vi "MainProgram.vi"(0 "DAQmx Task":refnum<k21>, 1 "BNC Port":refnum<visa-resource-name>, 2 "SRS Port":refnum<visa-resource-name>, 3 "Energy Meter  port":refnum<visa-resource-name>, 4 "SDG II port":refnum<visa-resource-name>, 5 "Mode":T18=enum."GenericTOF", 6 "Micos Port":refnum<visa-resource-name>="COM3", 7 "CommPort (ESP300)":refnum<visa-resource-name>="COM7", 8 "Serial Config (Micos)":T15={"Baud Rate"=115200, "Parity"=0, "Data Bits"=8, "Stop Bits"=10, "Flow Control"=0} {"Flow Control" items=["None", "XON/XOFF", "RTS/CTS", "XON/XOFF & RTS/CTS", "DTR/DSR", "XON/XOFF & DTR/DSR"]; "Stop Bits" items=["1.0"=10, "1.5"=15, "2.0"=20]; "Data Bits" items=["7"=7, "8"=8]; "Parity" items=["None", "Odd", "Even", "Mark", "Space"]; "Baud Rate" items=["300"=300, "600"=600, "1200"=1200, "2400"=2400, "4800"=4800, "9600"=9600, "19200"=19200]}, 9 "Serial Config (ESP300)":T15={"Baud Rate"=19200, "Parity"=0, "Data Bits"=8, "Stop Bits"=10, "Flow Control"=2} {"Flow Control" items=["None", "XON/XOFF", "RTS/CTS", "XON/XOFF & RTS/CTS", "DTR/DSR", "XON/XOFF & DTR/DSR"]; "Stop Bits" items=["1.0"=10, "1.5"=15, "2.0"=20]; "Data Bits" items=["7"=7, "8"=8]; "Parity" items=["None", "Odd", "Even", "Mark", "Space"]; "Baud Rate" items=["300"=300, "600"=600, "1200"=1200, "2400"=2400, "4800"=4800, "9600"=9600, "19200"=19200]}, 10 "#Axis (Micos)":i32=3, 11 "#Axis (ESP300)":i32=3, 12 "Simulation (Micos)":bool=TRUE, 13 "Simulation (ESP300)":bool=TRUE, 14 "MainDAQ_Selector":T16=enum."FakeSignal(Emulator)" caption="Restart Required", 15 "Laser Control Method":T17=enum."SDG_II" caption="Restart Required") -> ()   [LabVIEW 2013]
uses:
  Files/Signal_Segment.ctl
  ControlDef/ProcessingMode.ctl
  ControlDef/Average#.ctl
  ProcessMethods/Binning/BinType.ctl
  ControlDef/MainDAQ_Selector.ctl
  ControlDef/LaserCtrl_Method.ctl
  ControlDef/SpecLengthSelector.ctl
  ControlDef/SampleRateSelector.ctl
  ControlDef/DAQRangeSelector.ctl
  <instrlib>/DG535/Command/DG535_TriggerMode.ctl
  ControlDef/StepWidthSelector.ctl
  ControlDef/Files_Format.ctl
  <instrlib>/DG535/DG535_Configs.ctl
  <instrlib>/DG535/Command/Set Trigger.ctl
  <instrlib>/DG535/Command/Set Delay.ctl
  <instrlib>/DG535/Command/DG535_Channel.ctl
  <instrlib>/DG535/Command/Set Output.ctl
  <instrlib>/DG535/Command/DG535_Output.ctl
  <instrlib>/AnalogDiscSDKLv/VIs/DWF_AnalogIn_Configurations.ctl
  <instrlib>/AnalogDiscSDKLv/VIs/DWF_AcqMode.ctl
  <instrlib>/AnalogDiscSDKLv/VIs/DWF_Filter.ctl
  <instrlib>/AnalogDiscSDKLv/VIs/DWF_TrigSrc.ctl
  <instrlib>/AnalogDiscSDKLv/VIs/DWF_TrigCond.ctl
  <instrlib>/AnalogDiscSDKLv/VIs/DWF_TrigType.ctl
  <instrlib>/GageLv_uic/VI/Gage_Configs.ctl
  ControlDef/InstruMode_Typedef.ctl
  Hardware/BNC(QuantumComposers)/BNC_Configs.ctl
  ControlDef/InstrumentSpecificControls/UIC-AToF/InitializationParams_BNC565_2Ch_AToF.ctl
  Hardware/BNC(QuantumComposers)/Command/Set C-Input.ctl
  Hardware/BNC(QuantumComposers)/Command/Set C-Mode.ctl
  Hardware/BNC(QuantumComposers)/Command/Set C-Output.ctl
  Hardware/BNC(QuantumComposers)/Command/Set C-Enable.ctl
  <instrlib>/GenericDAQ/VI/GenericDAQ_Configs.ctl
  <vilib>/Utility/error.llb/DialogType.ctl
  ControlDef/AllControlsRefs.ctl
  ControlDef/States-AToF.ctl
  Hardware/FemtoLaser(Legacy)/Laser_Status.ctl
  Files/SaveControlsRef.ctl
  Files/WriterState.ctl
  Hardware/DAQmx(Legacy)/DAQmx_Status.ctl
  Hardware/EPM2000(Legacy)/EPM2K_Status.ctl
  ProcessMethods/SignalAverager/ProcessParams.ctl
  ProcessMethods/SignalAverager/DAQParams.ctl
  ProcessMethods/SignalAverager/DisplayGraph.ctl
  <instrlib>/ESP300/Public/Data/ESP300_State.ctl
  Hardware/BNC(QuantumComposers)/BNC_States.ctl
  <instrlib>/DG535/Command/DG535_States.ctl
  <instrlib>/Micos_uic/Public/Data/Micos_Data.ctl
  ControlDef/QueueRefs.ctl
  <instrlib>/AnalogDiscSDKLv/VIs/DWF_CtrlQueue.ctl
  <instrlib>/AnalogDiscSDKLv/VIs/DWF_State.ctl
  ControlDef/Signal.ctl
  ProcessMethods/SignalAverager/ProcessStates.ctl
  <instrlib>/AnalogDiscSDKLv/VIs/DWF_Signal.ctl
  <instrlib>/AnalogDiscSDKLv/VIs/DWF_PrivateStats.ctl
  <instrlib>/AnalogDiscSDKLv/VIs/DWF_InstrumentStatus.ctl
  <instrlib>/GageLv_uic/VI/Gage_PrivateStats.ctl
  <instrlib>/GageLv_uic/VI/Gage_DAQStatus.ctl
  Apps/GenericUSBCamera/CameraEventTypedef.ctl
  Hardware/Joystick/Joystick_UserEvent.ctl
  <instrlib>/GenericDAQ/VI/GenericDAQ_PrivateStats.ctl
  <instrlib>/GenericDAQ/VI/GenericDAQ_Status.ctl
  <instrlib>/GageLv_uic/VI/SetSecondaryDataVIRef_Typedef.ctl
  Files/BinaryHeader.ctl
  Apps/BeamProfiling/BeamProfiling_Params.ctl
  Apps/ImagingMS/Imaging_Params.ctl
  <instrlib>/Micos_uic/Public/Data/Micos_State.ctl
  <vilib>/Analysis/baseanly.llb/A x Vector.vi
  ControlDef/QuitProg.vi
  <instrlib>/Micos_uic/Public/Position_Micos.vi
  <instrlib>/ESP300/Public/Position_ESP300.vi
  ControlDef/MiscParams.vi
  ControlDef/PauseMeander.vi
  <userlib>/_OpenG.lib/comparison/comparison.llb/DBL Changed__ogtk.vi
  UI/Autoscale_Y_Single.vi
  <vilib>/Analysis/Matrix/Numeric/Conversions/Array To Matrix - RA2.vi
  <instrlib>/DG535/SRS_DG535_Lib.lvlib
  <instrlib>/ESP300/ESP300.lvlib
  <instrlib>/Micos_uic/Micos_uic.lvlib
  <userlib>/Utility/ErrorLog_lib.lvlib
  Hardware/Signal_Emulator(Legacy)/Emu_CoreDAQ_Globle.vi
  <instrlib>/AnalogDiscSDKLv/AnalogDiscSDKLv.lvlib
  <instrlib>/GageLv_uic/Gage.lvlib
  <vilib>/userdefined/High Color/IMAQdx.ctl
  <vilib>/Analysis/Matrix/NI_Matrix.lvlib
  <vilib>/Analysis/NI_AALBase.lvlib
  <instrlib>/GenericDAQ/GenericDAQ.lvlib
panel:
  out "Graph (B)":cluster{dbl[], dbl[]}(graph) caption="ChiMS, (C) 2014, Laser Ablation Time-of-Flight Mass Spectrometer with Postionization, under LGPLv3 license, rev.1845"
  in  "Scale(B)Y--":bool caption="AutoScale Y"
  in  "Scale(B)Y++":bool caption="AutoScale Y"
  in  "Binning(B)":bool
  in  "IncrementUpdate(B)":bool=TRUE caption="Increment"
  in  "Scale(B)X++":bool caption="AutoScale X"
  in  "Scale(B)X--":bool caption="AutoScale X"
  in  "Scale(B)_X":bool caption="AutoScale X"
  in  "GraphEnable (B)":bool=TRUE caption="Graph (B)"
  in  "Scale(B)_Y":bool caption="AutoScale Y"
  in  "SW_Average":T1=10 caption="Average" items=["1"=1, "5"=5, "10"=10, "25"=25, "50"=50, "100"=100, "250"=250, "500"=500, "1000"=1000, "2500"=2500, "5000"=5000]
  out "Graph (A)":cluster{dbl[], dbl[]}(graph)
  in  "Scale(A)Y--":bool caption="AutoScale Y"
  in  "Scale(A)Y++":bool caption="AutoScale Y"
  in  "Binning(A)":bool
  in  "IncrementUpdate(A)":bool caption="Increment"
  in  "Scale(A)X++":bool caption="AutoScale X"
  in  "Scale(A)X--":bool caption="AutoScale X"
  in  "Scale(A)_X":bool caption="AutoScale X"
  in  "Scale(A)_Y":bool caption="AutoScale Y"
  in  "GraphEnable (A)":bool=TRUE caption="Graph (A)"
  out "Nd:YAG Energy":dbl(slide) caption="Nd:YAG Energy (J)" scale=0.0..0.03 scale format="%#_2p"
  out "LaserEnergy":dbl(slide) caption="Spitfire Energy (J)" scale=0.0..2e-06 scale format="%#_2p"
  in  "LaserON":bool caption="Spitfire"
  in  "Files Format":T2=enum."Binary Files"
  in  "Snap":bool
  in  "Record":bool
  in  "Signal Segment":T3={"SampleRate"=1000000000.0, "TrigDelay"=0.0, "SpecLength"=512.0, "DAQ_Range"=1000.0, "Average#"=0, "Position"=[], "Spectrum"=[], "Calibr."=[], "Pressure"=-1.0, "Desp_LaserEnergy"=0.0, "PI_LaserEnergy"=0.0, "Voltages Table"=[[0.0, 0.0, 0.0, 0.0]], "ProcMode"=enum."None", "Threshold"=0.005, "Comment"="", "TickCount"=0.0, "Time Stamp"=timestamp(0 s since 1904-01-01)} {"TickCount" format="%#.2f"}
  in  "Setting Panel":T5(tab)=enum."Com.Setup"
  in  "Pause":bool
  in  "StepWidth (Micos)":T6=0.2 caption="StepWidth" items=["0.2 um"=0.0002, "0.001 mm"=0.001, "0.002 mm"=0.002, "0.005 mm "=0.005, "0.01 mm"=0.01, "0.02 mm"=0.02, "0.05 mm"=0.05, "0.1 mm"=0.1, "0.2 mm"=0.2, "1 mm"=1.0]
  in  "SetFocus":bool caption="Go To"
  in  "Focus (-)":bool
  in  "Focus (+)":bool
  in  "Back(+)":bool
  in  "Front(-)":bool
  in  "Back":bool
  in  "Front":bool
  in  "Down(-)":bool
  in  "Right(-)":bool
  in  "Up(+)":bool
  in  "Left(+)":bool
  in  "Right":bool
  in  "Left":bool
  in  "StopMoving":bool
  in  "Up":bool
  in  "Down":bool
  in  "Home(Micos)":bool
  in  "MoveAbs(Micos)":bool caption="Go To"
  in  "Destination":dbl[](array[numeric])=[17.0, 17.0, 24.2] caption="Destination (mm)" min=0.0 max=34.0 format="%#.5f"
  in  "Meander":bool
  in  "Accele.(Micos)":dbl=20.0 caption="Acceleration" format="%#.3f"
  in  "Velocity(Micos)":dbl=10.0 caption="Velocity" format="%#2.3f"
  out "Velcoty_ind_micos":dbl=10.0 caption="Velocity" format="%#_5f"
  out "Accele._ind_micos":dbl=20.0 caption="Acceleration" format="%#_4f"
  out "Position(Micos)":dbl[](array[numeric]) caption="Stage Position (mm)" format="%#.5f"
  in  "DepthProfile":bool
  in  "BeamProfiling(ESP)":bool
  in  "Velocity (ESP) #3":dbl=2.0 caption="Velocity#3" format="%#.3g"
  in  "DelayScan":bool
  in  "MotorDisabled(ESP)":bool
  in  "Meander (ESP)":bool
  in  "Accele. (ESP)":dbl=0.8 caption="Acceleration" format="%#.3g"
  in  "Set dbl pulse Delay":bool
  in  "DP_Delay (ps)":dbl caption="Delay (ps)" min=-3.0 max=300.0 format="%#.3f"
  in  "Down(ESP)":bool
  in  "Up(ESP)":bool
  in  "STOP(ESP)":bool
  in  "Left(ESP)":bool
  in  "Right(ESP)":bool
  in  "Destination(ESP)":dbl[](array[numeric])=[0.0, 0.25, 32.7] caption="Destination" min=0.0 max=360.0 format="%.4f"
  in  "Go(ESP)":bool
  in  "HomeSearch(ESP)":bool
  in  "Velocity (ESP)":dbl=0.2 caption="Velocity" format="%#.3g"
  out "Position(ESP)":dbl[](array[numeric]) caption="Currrent Postion"
  in  "StepWidth (ESP)":T6=0.1 caption="StepWidth (mm)" items=["0.2 um"=0.0002, "0.001 mm"=0.001, "0.002 mm"=0.002, "0.005 mm "=0.005, "0.01 mm"=0.01, "0.02 mm"=0.02, "0.05 mm"=0.05, "0.1 mm"=0.1, "0.2 mm"=0.2, "1 mm"=1.0]
  in  "ZeroDelayPos":dbl=0.679 caption="0 Delay@(mm)" format="%#.3f"
  out "DP_Delay (ps)_indicator":dbl caption="Delay (ps)" min=-3.0 max=300.0 format="%#.3f"
  in  "Delay(PI)":dbl=3e-05 caption="VUV Delay" min=-0.001 max=0.001 step=1e-08 format="%_3ps"
  in  "Delay(LDI-Rej.)":dbl=-2e-06 caption="LDIRej_end" min=-0.001 max=0.0 step=1e-07 format="%_3ps"
  in  "SRS On/Off":bool caption="Dont Rely On\nShowing\nCheck BNC"
  in  "Internal/Burst Rate":dbl=10.0 caption="Internal/Burst Rate (Hz)" min=0.001 max=1000000.0 format="%.3f"
  in  "Trigger Mode (SRS)":T7=enum."External" caption="Trigger Mode"
  in  "Ch_D":dbl=2.8e-05 format="%_3ps"
  in  "Ch_C":dbl format="%_3ps"
  in  "Ch_B":dbl=3e-05 format="%_3ps"
  in  "Ch_A":dbl=0.099807701 format="%_7ps"
  in  "Width B":dbl=1e-06 min=0.0 max=9.9e-05 step=1e-09 format="%_3ps"
  in  "Width A":dbl=1e-06 min=0.0 max=9.9e-05 step=1e-09 format="%_3ps"
  in  "BNC On/Off":bool caption="Dont Rely On\nShowing\nCheck BNC"
  in  "Mode (BNC)":T8(ring)=enum."Single Shot" caption="Mode"
  in  "Channels Enable Status":bool[](array[boolean])=[TRUE, TRUE]
  in  "Set Mode":bool caption="Set BNC"
  in  "Trigger Mode (BNC)":T9(ring)=enum."Triggered" caption="Trigger Mode"
  in  "Rep.Rate (BNC)":dbl=10.0 caption="Repetive Rate" min=0.0 max=1000.0 format="%#_6f Hz"
  in  "Delay B":dbl min=0.0 max=9.9e-05 step=1e-09 format="%_3ps"
  in  "Delay A":dbl format="%_3ps"
  in  "Gain (Voltage Range)":T10=4294966296 items=["-100~900 mV"=4294966296, "-380~20 mV"=4294966895, "-20~380 mV"=4294966896, "+/-5 V"=10000, "+/-2 V"=4000, "+/-1 V"=2000, "+/-500 mV"=1000, "+/-200 mV"=400, "+/-100 mV"=200, "+/-50 mV"=100]
  in  "Spectrum Length":T11=32768.0 items=["256K"=262144.0, "192K"=196608.0, "128K"=131072.0, "96K"=98304.0, "64K"=65280.0, "32K"=32768.0, "24K"=24576.0, "16K"=16384.0, "8K"=8192.0, "1K"=1024.0, "512"=512.0]
  in  "SampleRate":T12=500000000.0 items=["50MS/s"=50000000.0, "100MS/s"=100000000.0, "125MS/s"=125000000.0, "200MS/s"=200000000.0, "250MS/s"=250000000.0, "500MS/s"=500000000.0, "1GS/s"=1000000000.0, "1.6GS/s"=1600000000.0]
  in  "Threshold":dbl=0.01 format="%#_3pV"
  in  "Baseline":dbl
  in  "TopLine":dbl=1.0
  in  "Processing Mode":T4
  in  "ZeroOffsetCorrection":dbl=0.0055 format="%.3p V"
  in  "Resolution(B)":bool
  in  "Resolution(A)":bool
  in  "Cali.":dbl[](array[numeric])=[0.0707, 0.16163, 0.02539] caption="Calibration Params (a, b, c)" format="%#.6f"
  in  "Switch(SDG_II)":bool caption="Status"
  in  "Mode(SDG_II)":bool caption="Mode"
  in  "ManlTrig(SDG)":bool caption="Manual Trigger"
  in  "BinWidth (A)":dbl=0.1
  in  "BinType (A)":T13=enum."ByMass"
  in  "BinWidth (B)":dbl=0.5
  in  "BinType (B)":T13=enum."ByScreen"
  in  "DisplayIncrement":u32=15
  in  "YAGEnergyCoeff.":dbl=132.6
  in  "fsEnergyCoeff.":dbl=1.29
  in  "GenericDAQ_Config":T14={"Acquisition"={"Sample Rate"=1000000000.0, "Mode"=0, "Start (0)"=0.0, "Depth"=1024.0, "Segment"=1}, "Channels"=[{"Range"=1, "DC Offset"=0}], "Mode(Gage)"=enum."Continuous"} {"Acquisition"."Depth" min=256.0 step=128.0; "Acquisition"."Mode" items=["Single", "Dual", "Quad", "Octal"]; "Acquisition"."Sample Rate" format="%.0p"}
  out "Filename Indicator":path caption="Filename"
  in  "ComSettingsTab":enum32{"Micos", "ESP300", "Misc", "Misc 2"}(tab)=enum."ESP300"
  in  "ColdStartReset":bool=TRUE caption="ResetSettings"
  in  "Gage_Config":T19={"Acquisition"={"Sample Rate"=500000000.0, "Mode"=0, "Start (0)"=0.0, "Depth"=32768.0, "Segment Size"=32768.0, "Trigger Delay"=0.0, "Trigger Timeout"=-1.0, "Trigger Holdoff"=0.0, "Clock mode"=enum."Internal", "Segment"=1}, "Channels"=[{"Coupling"=1, "Differential Input"=FALSE, "Direct-to-ADC"=FALSE, "Range"=2000, "Impedance"=50, "DC Offset"=0, "Filter"=0}], "Trigger"={"Slope"=1, "Level"=25, "Source"=0, "External Range"=10000, "External Coupling"=0, "External"=TRUE, "Disable"=FALSE, "External Impedance"=0}, "Mode(Gage)"=enum."Continuous"} {"Trigger"."External Impedance" items=["50 Ohm", "HiZ"]; "Trigger"."External Coupling" items=["DC", "AC"]; "Trigger"."External Range" min=2000 max=10000 step=8000; "Trigger"."Slope" items=["Rising", "Falling"]; "Trigger"."Level" min=-100 max=100; "Trigger"."Source" min=0 max=64 step=1; "Channels"."Impedance" min=50 max=1000000 step=999950; "Channels"."Coupling" items=["DC", "AC"]; "Acquisition"."Segment Size" min=256.0 step=128.0; "Acquisition"."Trigger Delay" min=0.0 step=128.0; "Acquisition"."Trigger Timeout" format="%.0p"; "Acquisition"."Trigger Holdoff" min=0.0 step=128.0; "Acquisition"."Depth" min=256.0 step=128.0; "Acquisition"."Mode" items=["Single", "Dual", "Quad", "Octal"]; "Acquisition"."Sample Rate" format="%.0p"}
  in  "AnalogDisc_Configs":T20={"Acqusition"={"Freq(Hz,SampleRate)"=10000000.0, "BufferSize"=8192, "Mode"=enum."Single", "RecordLength(s)"=8192.0}, "Channels"=[{"Range(V)"=5.0, "Offset(V)"=0.0, "Filter"=enum."Decimate", "Enable"=TRUE}], "Trigger"={"TriggerSource"=enum."None", "Timeout(s)"=0.0, "Holdoff(s)"=1e-06, "Position(s)"=0.0}, "AnalogTrigger"={"Channel"=0, "Polarity"=enum."Rising", "Type"=enum."Pulse", "Level(V)"=0.0, "Filter"=enum."Decimate", "Hysterisis(V)"=0.0}} {"AnalogTrigger"."Hysterisis(V)" format="%#_6p"; "Acqusition"."RecordLength(s)" format="%#_6p"; "Acqusition"."Freq(Hz,SampleRate)" format="%#_6p"; "Acqusition"."BufferSize" min=1 max=16384 step=1; "Trigger"."Position(s)" format="%#_6p"; "Trigger"."Holdoff(s)" format="%#_6p"}
  in  "Timing Tab":enum32{"DG535", "BNC"}(tab)
  in  "DG535_Configs":T26={"Trigger"={"Trigger Mode"=enum."External", "Internal/Burst Rate"=10.0, "External  Level"=1.5, "Impedance"=TRUE, "Slope"=FALSE}, "Delays"=[{"Channel"=enum."A Output", "Sync To"=enum."T0 Output", "Delay"=0.099807701}, {"Channel"=enum."B Output", "Sync To"=enum."A Output", "Delay"=1.2e-05}, {"Channel"=enum."C Output", "Sync To"=enum."T0 Output", "Delay"=0.0}, {"Channel"=enum."D Output", "Sync To"=enum."T0 Output", "Delay"=1e-05}, {"Channel"=enum."Trigger Input", "Sync To"=enum."T0 Output", "Delay"=0.0}], "Output"=[{"Channel"=enum."A Output", "Level"=enum."TTL", "Load"=TRUE, "Polarity"=FALSE, "Amplitude"=1.0, "Offset"=0.0}, {"Channel"=enum."B Output", "Level"=enum."TTL", "Load"=FALSE, "Polarity"=TRUE, "Amplitude"=1.0, "Offset"=0.0}, {"Channel"=enum."C Output", "Level"=enum."TTL", "Load"=TRUE, "Polarity"=FALSE, "Amplitude"=1.0, "Offset"=0.0}, {"Channel"=enum."D Output", "Level"=enum."TTL", "Load"=TRUE, "Polarity"=FALSE, "Amplitude"=1.0, "Offset"=0.0}, {"Channel"=enum."T0 Output", "Level"=enum."TTL", "Load"=FALSE, "Polarity"=FALSE, "Amplitude"=1.0, "Offset"=0.0}, {"Channel"=enum."AB Output", "Level"=enum."TTL", "Load"=TRUE, "Polarity"=FALSE, "Amplitude"=1.0, "Offset"=0.0}, {"Channel"=enum."CD Output", "Level"=enum."TTL", "Load"=TRUE, "Polarity"=FALSE, "Amplitude"=1.0, "Offset"=0.0}]} caption="DG535 Settings (Restart Needed)" {"Trigger"."External  Level" min=-2.56 max=2.56 format="%.2f"; "Trigger"."Internal/Burst Rate" min=0.001 max=1000000.0 format="%.3f"; "Delays"."Delay" format="%#_6p"; "Output"."Offset" min=-3.0 max=4.0 format="%.2f"; "Output"."Amplitude" min=-3.0 max=4.0 format="%.2f"}
  in  "BNC_Config":T32={"System"={"Rep.Rate"=1000.0, "Sys Ext Mode"=enum."Triggered", "Mode"=enum."Single Shot"}, "Channels"=[]}
  in  "CameraOn":bool caption="Go To"
  out "Info":string="subProgram Ready..."
  out "Write Counter":i32
  out "Trig. Rate (Hz)":dbl=88.0 caption="DAQ Rate" format="%#.1p"
  out "Moving (Newport)":bool
  out "Moving (Micos)":bool
  in  "Quit":bool
  # "(C) 2014 UIC, Yang Cui, Luke Hanley. Provided AS IS, use at your own risk."
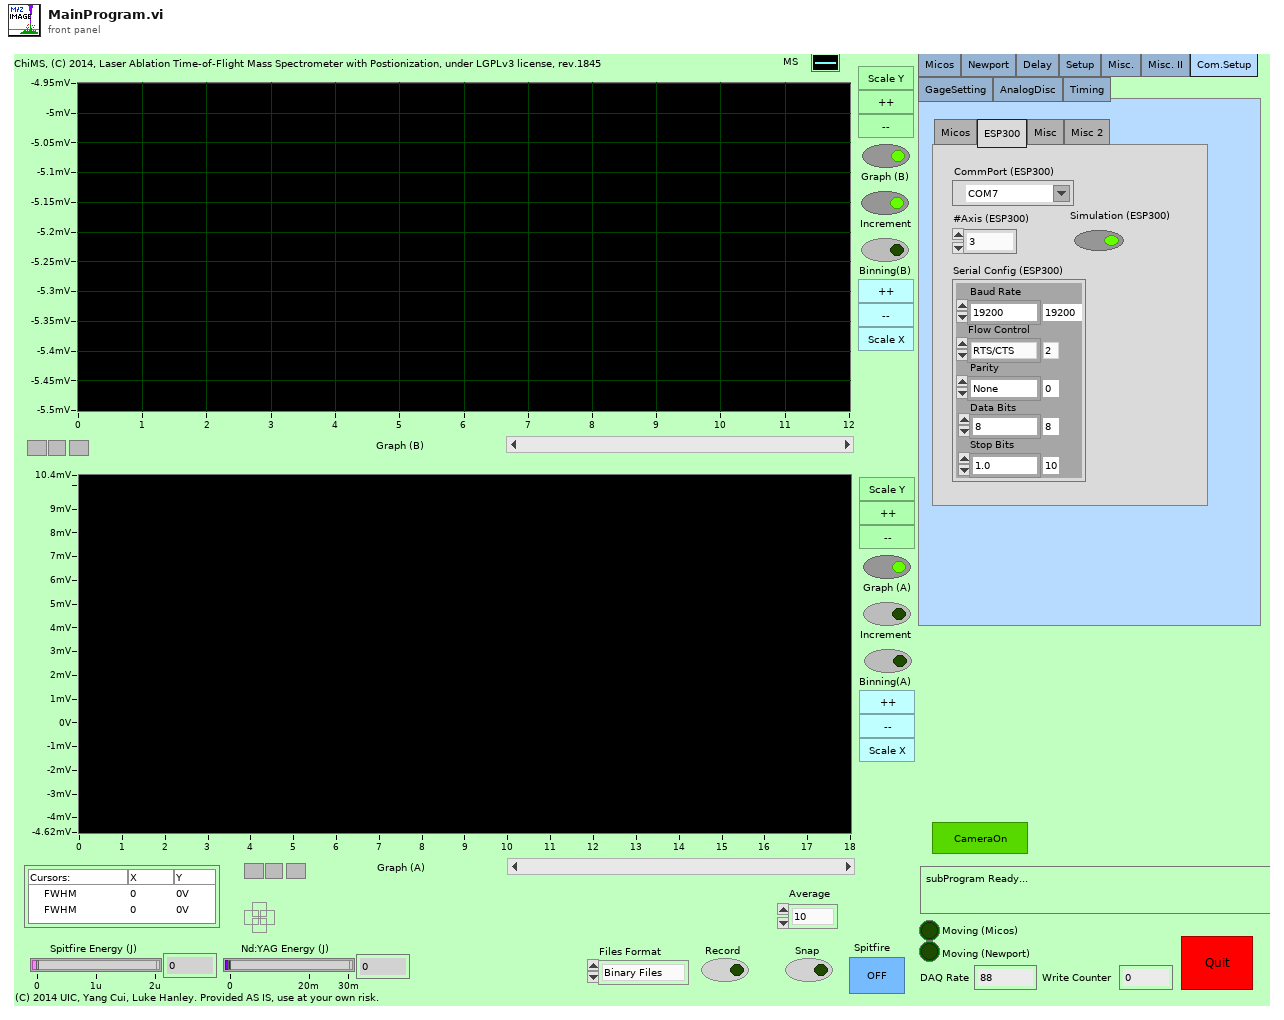
[diagram p1: front panel]
types:
  T1 = typedef "Average#.ctl" = u16
  T2 = typedef "Files_Format.ctl" = enum16{"Text Files", "mzML Files", "Binary Files", "BioMap Files", "imzML Files"}
  T3 = typedef "Signal_Segment.ctl" = cluster{"SampleRate":dbl, "TrigDelay":dbl, "SpecLength":dbl, "DAQ_Range":dbl, "Average#":i32, "Position":dbl[], "Spectrum":sgl[], "Calibr.":dbl[], "Pressure":dbl, "Desp_LaserEnergy":dbl, "PI_LaserEnergy":dbl, "Voltages Table":sgl[][], "ProcMode":T4, "Threshold":dbl, "Comment":string, "TickCount":dbl, "Time Stamp":timestamp}
  T4 = typedef "ProcessingMode.ctl" = enum16{"None", "Drop by Threshold", "TDC Simulate", "SetFilter"}
  T5 = enum32{"Micos", "Newport", "Delay", "Setup", "Misc.", "Misc. II", "Com.Setup", "GageSetting", "AnalogDisc", "Timing"}
  T6 = typedef "StepWidthSelector.ctl" = dbl
  T7 = typedef "SRS_DG535_Lib.lvlib/DG535_TriggerMode.ctl" = enum16{"Internal", "External", "SingleShot", "Burst", "Line"}
  T8 = enum16{"Normal", "Single Shot", "Duty Cycle", "Burst"}
  T9 = enum16{"Disabled", "Triggered", "Gated", "Triggered & Gated"}
  T10 = typedef "DAQRangeSelector.ctl" = u32
  T11 = typedef "SpecLengthSelector.ctl" = dbl
  T12 = typedef "SampleRateSelector.ctl" = dbl
  T13 = typedef "BinType.ctl" = enum16{"ByTime", "ByScreen", "ByMass", "ToUnitMass"}
  T14 = typedef "GenericDAQ.lvlib/GenericDAQ_Configs.ctl" = cluster{"Acquisition":cluster{"Sample Rate":dbl, "Mode":u16, "Start (0)":dbl, "Depth":dbl, "Segment":u32}, "Channels":cluster{"Range":u32, "DC Offset":i32}[], "Mode(Gage)":enum16{"Normal", "Continuous", "MultiRecord", "HwAverage"}}
  T15 = cluster{"Baud Rate":u32, "Parity":u16, "Data Bits":u16, "Stop Bits":u16, "Flow Control":u16}
  T16 = typedef "MainDAQ_Selector.ctl" = enum16{"None", "Gage", "Gage_AdvMultiRec_8bit1Ch", "IonWerks_TDCx4", "Tektronics", "KnifeEdge_Emu", "AnalogDisc", "Gage_AMR_8bit2Ch", "Gage_AMR_16bit1Ch", "Gage_AMR_16bit2Ch", "FakeSignal(Emulator)"}
  T17 = typedef "LaserCtrl_Method.ctl" = enum16{"SRS_DG535", "BNC", "SDG_II"}
  T18 = typedef "InstruMode_Typedef.ctl" = enum16{"fsLDPI", "nsLDPI", "nsLD-fsPI", "GenericTOF", "BeamProfiling"}
  T19 = typedef "Gage.lvlib/Gage_Configs.ctl" = cluster{"Acquisition":cluster{"Sample Rate":dbl, "Mode":u16, "Start (0)":dbl, "Depth":dbl, "Segment Size":dbl, "Trigger Delay":dbl, "Trigger Timeout":dbl, "Trigger Holdoff":dbl, "Clock mode":enum16{"Internal", "External", "Reference"}, "Segment":u32}, "Channels":cluster{"Coupling":u16, "Differential Input":bool, "Direct-to-ADC":bool, "Range":u32, "Impedance":u32, "DC Offset":i32, "Filter":i32}[], "Trigger":cluster{"Slope":u16, "Level":i32, "Source":i32, "External Range":u32, "External Coupling":u16, "External":bool, "Disable":bool, "External Impedance":u16}, "Mode(Gage)":enum16{"Normal", "Continuous", "MultiRecord", "HwAverage"}}
  T20 = typedef "AnalogDiscSDKLv.lvlib/DWF_AnalogIn_Configurations.ctl" = cluster{"Acqusition":cluster{"Freq(Hz,SampleRate)":dbl, "BufferSize":i32, "Mode":T21, "RecordLength(s)":dbl}, "Channels":cluster{"Range(V)":dbl, "Offset(V)":dbl, "Filter":T22, "Enable":bool}[], "Trigger":cluster{"TriggerSource":T23, "Timeout(s)":dbl, "Holdoff(s)":dbl, "Position(s)":dbl}, "AnalogTrigger":cluster{"Channel":i32, "Polarity":T24, "Type":T25, "Level(V)":dbl, "Filter":T22, "Hysterisis(V)":dbl}}
  T21 = typedef "AnalogDiscSDKLv.lvlib/DWF_AcqMode.ctl" = enum16{"Single", "ScanShift", "ScanScreen", "Record"}
  T22 = typedef "AnalogDiscSDKLv.lvlib/DWF_Filter.ctl" = enum16{"Decimate", "Average", "MinMax"}
  T23 = typedef "AnalogDiscSDKLv.lvlib/DWF_TrigSrc.ctl" = enum16{"None", "PC", "DetectorAnalogIn", "DetectorDigitalIn", "AnalogIn", "DigitalIn", "DigitalOut", "AnalogOut1", "AnalogOut2", "AnalogOut3", "AnalogOut4", "External1", "External2", "External3", "External4"}
  T24 = typedef "AnalogDiscSDKLv.lvlib/DWF_TrigCond.ctl" = enum16{"Rising", "Falling"}
  T25 = typedef "AnalogDiscSDKLv.lvlib/DWF_TrigType.ctl" = enum16{"Edge", "Pulse", "Transition"}
  T26 = typedef "SRS_DG535_Lib.lvlib/DG535_Configs.ctl" = cluster{"Trigger":T27, "Delays":T28[], "Output":T30[]}
  T27 = typedef "SRS_DG535_Lib.lvlib/Set Trigger.ctl" = cluster{"Trigger Mode":T7, "Internal/Burst Rate":dbl, "External  Level":sgl, "Impedance":bool, "Slope":bool}
  T28 = typedef "SRS_DG535_Lib.lvlib/Set Delay.ctl" = cluster{"Channel":T29, "Sync To":T29, "Delay":dbl}
  T29 = typedef "SRS_DG535_Lib.lvlib/DG535_Channel.ctl" = enum16{"Trigger Input", "T0 Output", "A Output", "B Output", "AB Output", "C Output", "D Output", "CD Output", "NULL"}
  T30 = typedef "SRS_DG535_Lib.lvlib/Set Output.ctl" = cluster{"Channel":T29, "Level":T31, "Load":bool, "Polarity":bool, "Amplitude":dbl, "Offset":dbl}
  T31 = typedef "SRS_DG535_Lib.lvlib/DG535_Output.ctl" = enum16{"TTL", "NIM", "ECL", "Variable"}
  T32 = typedef "BNC_Configs.ctl" = cluster{"System":cluster{"Rep.Rate":dbl, "Sys Ext Mode":enum16{"Disabled", "Triggered", "Gated", "Triggered & Gated"}, "Mode":enum16{"Normal", "Single Shot", "Duty Cycle", "Burst"}}, "Channels":T33[]}
  T33 = typedef "InitializationParams_BNC565_2Ch_AToF.ctl" = cluster{"C-Input":T34, "C-Mode":T35, "C-Output":T36, "C-Enables":T37}
  T34 = typedef "Set C-Input.ctl" = cluster{"Channel":i32, "Sync Source":i32}
  T35 = typedef "Set C-Mode.ctl" = cluster{"Channel":i32, "Delay":dbl, "Width":dbl}
  T36 = typedef "Set C-Output.ctl" = cluster{"Channel":i32, "Polarity":bool}
  T37 = typedef "Set C-Enable.ctl" = cluster{"Channel":i32, "Enable":bool}
  T38 = typedef "AllControlsRefs.ctl" = cluster{"Communication":cluster{"Micos":cluster{"Simulation (Micos)":refnum<vi>, "Micos Port":refnum<vi>, "Serial Config (Micos)":refnum<vi>, "#Axis (Micos)":refnum<vi>}, "ESP300":cluster{"Simulation (ESP300)":refnum<vi>, "CommPort (ESP300)":refnum<vi>, "Serial Config (ESP300)":refnum<vi>, "#Axis (ESP300)":refnum<vi>}, "DAQmx Task":refnum<vi>, "BNC Port":refnum<vi>, "SRS Port":refnum<vi>, "SDG_II port":refnum<vi>, "EnergyMeter port":refnum<vi>}, "Method":cluster{"Mode":refnum<vi>, "MainDAQ_Selector":refnum<vi>, "LaserCtrlMethod":refnum<vi>}, "DG535":cluster{"Delay(PI)":refnum<vi>, "Delay(LDI-Rej.)":refnum<vi>, "Internal/Burst Rate":refnum<vi>, "Trigger Mode (SRS)":refnum<vi>}, "BNC":cluster{"Mode (BNC)":refnum<vi>, "Channels Enable Status":refnum<vi>, "Trigger Mode (BNC)":refnum<vi>, "Rep.Rate (BNC)":refnum<vi>, "Delay A":refnum<vi>, "Width A":refnum<vi>, "Delay B":refnum<vi>, "Width B":refnum<vi>}, "Expt":cluster{"Cali.":refnum<vi>, "Gain (Voltage Range)":refnum<vi>, "Spectrum Length":refnum<vi>, "SampleRate":refnum<vi>, "Processing Mode":refnum<vi>, "Threshold":refnum<vi>, "Baseline":refnum<vi>, "TopLine":refnum<vi>, "ZeroOffsetCorrection":refnum<vi>}, "LowLevel":cluster{"AnalogDisc_Configs":refnum<vi>, "DG535_Configs":refnum<vi>, "Gage_Config":refnum<vi>, "BNC_Config":refnum<vi>}}
  T39 = typedef "DialogType.ctl" = u16
  T40 = cluster{"AnalogDisc_Configs":refnum<vi>, "DG535_Configs":refnum<vi>, "Gage_Config":refnum<vi>, "BNC_Config":refnum<vi>}
  T41 = cluster{"Mode":refnum<vi>, "MainDAQ_Selector":refnum<vi>, "Laser Control Method":refnum<vi>}
  T42 = cluster{"Delay(PI)":refnum<vi>, "Delay(LDI-Rej.)":refnum<vi>, "Internal/Burst Rate":refnum<vi>, "Trigger Mode (SRS)":refnum<vi>}
  T43 = cluster{"Simulation (ESP300)":refnum<vi>, "CommPort (ESP300)":refnum<vi>, "Serial Config (ESP300)":refnum<vi>, "#Axis (ESP300)":refnum<vi>}
  T44 = cluster{"Simulation (Micos)":refnum<vi>, "Micos Port":refnum<vi>, "Serial Config (Micos)":refnum<vi>, "#Axis (Micos)":refnum<vi>}
  T45 = cluster{"Mode (BNC)":refnum<vi>, "Channels Enable Status":refnum<vi>, "Trigger Mode (BNC)":refnum<vi>, "Rep.Rate (BNC)":refnum<vi>, "Delay A":refnum<vi>, "Width A":refnum<vi>, "Delay B":refnum<vi>, "Width B":refnum<vi>}
  T46 = cluster{"Cali.":refnum<vi>, "Gain (Voltage Range)":refnum<vi>, "Spectrum Length":refnum<vi>, "SampleRate":refnum<vi>, "Processing Mode":refnum<vi>, "Threshold":refnum<vi>, "Baseline":refnum<vi>, "TopLine":refnum<vi>, "ZeroOffsetCorrection":refnum<vi>}
  T47 = cluster{cluster{"Simulation (Micos)":refnum<vi>, "Micos Port":refnum<vi>, "Serial Config (Micos)":refnum<vi>, "#Axis (Micos)":refnum<vi>}, cluster{"Simulation (ESP300)":refnum<vi>, "CommPort (ESP300)":refnum<vi>, "Serial Config (ESP300)":refnum<vi>, "#Axis (ESP300)":refnum<vi>}, "DAQmx Task":refnum<vi>, "BNC Port":refnum<vi>, "SRS Port":refnum<vi>, "SDG II port":refnum<vi>, "Energy Meter  port":refnum<vi>}
  T48 = cluster{"Trigger":T27, "Delays":T28[], "Output":T30[]}
  T49 = enum8{"Enabled", "Disabled", "Disabled and Grayed Out"}
  T50 = typedef "InstrumentConfiguration.ctl" = cluster{"Mode":string, "InstrumentMode":cluster{"MainDAQ_Selector":T16, "LaserCtrlMethod":T17, "InstruMode":T18}, "CommuniationSettings":cluster{"SDG_II":refnum<visa-resource-name>, "DG535":refnum<visa-resource-name>, "BNC565":refnum<visa-resource-name>, "EPM2000":refnum<visa-resource-name>, "NI-DAQmx":refnum<visa-resource-name>, "Micos":cluster{"Simulation":bool, "ComPort":refnum<visa-resource-name>, "Serial Config":cluster{"Baud Rate":u32, "Parity":u16, "Data Bits":u16, "Stop Bits":u16, "Flow Control":u16}, "#Axis":i32}, "ESP300":cluster{"Simulation":bool, "ComPort":refnum<visa-resource-name>, "Serial Config":cluster{"Baud Rate":u32, "Parity":u16, "Data Bits":u16, "Stop Bits":u16, "Flow Control":u16}, "#Axis":i32}}, "DG535":cluster{"Trigger":T27, "Delays":T28[], "Output":T30[]}, "Gage_Config":T19, "AnalogDisc_Config":T20, "Micos":cluster{"Velocity":dbl, "Acceleration":dbl}, "ESP300":cluster{"Velocity":dbl[], "Acceleration":dbl[]}, "EPM2000":cluster{"Factor(A)":dbl, "Factor(B)":dbl}, "ProcessMethod":cluster{"TopLine":dbl, "Threshold":dbl, "Baseline":dbl, "ZeroOffset":dbl, "Processing Mode":T4}, "Timing(LDPI)":cluster{"Delay(PI)":dbl, "Delay(Rejection)":dbl, "NoDelayOffset":dbl, "RepRate(Hz)":dbl}, "Cali.":dbl[], "BNC_Config":T32}
  T51 = typedef "GenericDAQ.lvlib/GenericDAQ_PrivateStats.ctl" = cluster{"Model":string, "TrigRate(Hz)":dbl, "TrigCount":i32, "Mode":enum16{"Normal", "Continuous", "MultiRecord", "HwAverage"}, "DAQ_Status":T52, "SecondaryDataVIRef":refnum<vi>, "Option(SecondaryDataVI)":i32, "cSegment":i32}
  T52 = typedef "GenericDAQ.lvlib/GenericDAQ_Status.ctl" = enum16{"Done", "Armed", "Triggered", "Transfering"}
  T53 = typedef "Joystick_UserEvent.ctl" = cluster{"StepMove":refnum<user-event>, "ContMove":refnum<user-event>, "EStop":refnum<user-event>}
  T54 = typedef "CameraEventTypedef.ctl" = cluster{"Command":enum16{"MouseClick", "MouseDoubleClick", "MouseRightClick", "SetCalibration", "AutoCalibration"}, "Params.":variant}
  T55 = typedef "Gage.lvlib/Gage_PrivateStats.ctl" = cluster{"Model":string, "TrigRate(Hz)":dbl, "TrigCount":i32, "Mode(Gage)":enum16{"Normal", "Continuous", "MultiRecord", "HwAverage"}, "Handle":cluster{"Handle":u32, "Sample size":u32, "Resolution":i32, "Offset":i32, "Channels":u32, "Boards":u32}, "DAQ_Status":T56, "SecondaryDataVIRef":refnum<vi>, "Option(SecondaryDataVI)":i32, "cSegment":i32, "TSArray":dbl[], "Adj.SegmenttSize":dbl}
  T56 = typedef "Gage.lvlib/Gage_DAQStatus.ctl" = enum16{"Done", "Armed", "Triggered", "Transfering"}
  T57 = typedef "AnalogDiscSDKLv.lvlib/DWF_PrivateStats.ctl" = cluster{"Handle_DWF":i32, "Model":string, "SN":string, "TrigRate(Hz)":dbl, "TrigCount":i32, "Mode":enum16{"Normal", "Turbo"}, "STS":T58, "SecondaryDataParams.":cluster{"SecondaryDataVIRef.":refnum<vi>, "Option":i32}}
  T58 = typedef "AnalogDiscSDKLv.lvlib/DWF_InstrumentStatus.ctl" = enum16{"stsRdy", "stsARM", "stsDone", "stsTrig", "stsCfg", "stsPrefill", "stsNotDone", "stsTrigDly", "stsError", "stsBusy", "stsStop"}
  T59 = typedef "AnalogDiscSDKLv.lvlib/DWF_Signal.ctl" = cluster{"tickcount":u32, "Signal":sgl[][], "SecondaryData":dbl[], "Flag":enum16{"Normal", "MultiRecStart", "MultiRecEnd", "Reserved1", "Reserved2", "Reserved3"}}
  T60 = typedef "AnalogDiscSDKLv.lvlib/DWF_CtrlQueue.ctl" = cluster{"DWF States":T61, "Variant":variant}
  T61 = typedef "AnalogDiscSDKLv.lvlib/DWF_State.ctl" = enum16{"Enumerate", "Open", "Close", "CloseAll", "Reset", "Quit", "==Settings==", "SetAcquisition_", "SetChannels_", "SetTrigger_", "SetAnalogTrigDetector_", "SetAll_AcquChTrig_", "fConfigurate", "fStart", "GetStatus", "_WaitForDone/Idle", "_GetData", "GetAcquisition", "GetChannels", "GetTrigger", "GetAll_AcquChTrig", "==Messaging==", "_PushDataOut", "GetStat_", "GetConfig_", "==ModeSetup==", "SetSignalBuffer_", "SetMode_", "SetSecondaryDataRef._", "==AnalogOut==", "GetChannelCount_AO", "fStart_AO", "SetChEnable_AO", "SetConfig_AO", "SetFuncData_AO", "SetOffset_AO_", "SetMasterNode_AO", "SetStates_AO", "SetSymetry_AO", "SetTriggerSource_AO", "==Trigger==", "ManualTrigger"}
  T62 = typedef "QueueRefs.ctl" = cluster{"LaserCtrlMethod":T17, "Apps":refnum<queue>, "MainDAQCoreQueue":refnum<queue>, "Micos":refnum<queue>, "ESP300":refnum<queue>, "SMC100":refnum<queue>, "SRS DG535":refnum<queue>, "BNC":refnum<queue>, "SDG_ii":refnum<queue>, "NI-USB_DAQmx":refnum<queue>, "ProcCore_CtrlQueue":refnum<queue>, "WriterCtrl":refnum<queue>, "WriterSIG":refnum<queue>, "Feedback":refnum<queue>, "EPM2000":refnum<queue>, "InfoRef":refnum<vi>, "AppsLock":T63, "ProcCore_SignalQueue":refnum<queue>}
  T63 = typedef "Semaphore RefNum" = refnum<k1>
  T64 = typedef "Micos_uic.lvlib/Micos_Data.ctl" = cluster{"Position":dbl[], "Velocity":dbl[], "Acceleration":dbl[], "Moving":bool, "Simulation":bool, "tickcount_mov":u32, "tickcount_pos":u32, "NumOfAxis":i32, "Initialized":bool, "CommPort":refnum<visa-resource-name>, "Range":dbl[][], "Serial Configuration":cluster{"Baud Rate":u32, "Parity":u16, "Data Bits":u16, "Stop Bits":u16, "Flow Control":u16}, "MotorDisabled":refnum<vi>}
  T65 = typedef "ProcessParams.ctl" = cluster{"DisplayIncrement":u32, "DisplayIncrementRef":refnum<vi>, "Rep .Rate (Hz)":dbl, "Save":bool, "SW_Average":u32, "Filter":T4, "FilterParams":variant, "DAQParams":T66, "Graph":T67[], "CmdParams.":variant, "Average(SW)Ref":refnum<vi>, "Calibr.Params":refnum<vi>, "SignalSegmentRef":refnum<vi>, "WriterQueue":refnum<queue>}
  T66 = typedef "DAQParams.ctl" = cluster{"TrigDelay":dbl, "Offset":i32, "Resolution":i32, "Range (mV)":u32, "Sample Rate":dbl, "Depth":dbl, "Segments":u32}
  T67 = typedef "DisplayGraph.ctl" = cluster{"XY_Graph":refnum<vi>, "Enable":bool, "IncreDisplay":bool, "Binning":bool, "IncremetDisplayRef":refnum<vi>, "PlotDisplayRef":refnum<vi>, "BinningRef":refnum<vi>, "FWHM":bool, "ResoltionRef":refnum<vi>, "BinWidthRef":refnum<vi>, "BinWidth":dbl, "BinTypeRef":refnum<vi>, "BinType":T13}
  T68 = typedef "WriterState.ctl" = cluster{"State":enum16{"Open", "Close", "ChangeFormat", "SetHeader", "QuitProg."}, "Params":variant}
  T69 = typedef "SaveControlsRef.ctl" = cluster{"Write Counter":refnum<vi>, "Segment Counter":refnum<vi>, "Writer error out":refnum<vi>}
  T70 = typedef "Laser_Status.ctl" = cluster{"State":enum16{"Initialize", "Idle/Update", "Configure", "Turn On", "Tun OFF", "Continuous", "Single Shot", "ManualTrigger", "Close", "Quit"}, "Parameter":dbl}
  T71 = typedef "States-AToF.ctl" = enum16{"Initialize", "Idle", "CalcMzArray", "Meander_SGL_MCS", "Meander_MCS", "CleanSurface", "Meander_Npt", "Meander_SGL_Npt", "KnifeEdgeExpt", "KnifeEdgeExpt_Npt", "Imaging_Micos", "Imaging_ESP", "DepthProfiling", "Set_2PulseDelay", "DelayScan", "PeakSearch", "ExportOrigin", "Save Settings", "Load Settings", "Save as Default", "Load Default", "EnergyCalibration", "Quit", "Interrupted_Stop", "Quit_SubProgram", "StepMove_Joystick", "ContMove_Joystick", "Stop_Joystick", "Check_AppsLock", "Return_Status", "DepthProfile_RT", "UpdateInstruStates", "InstruOptimizer_static", "InstruOptimizer_dynamic", "DepthProfiling(3D)"}
  T72 = typedef "SetSecondaryDataVIRef_Typedef.ctl" = cluster{"SecondaryDataVIRef.":refnum<vi>, "Option":i32}
  T73 = cluster{"SecondaryDataVIRef.":refnum<vi>, "Option":i32}
  T74 = typedef "ESP300.lvlib/ESP300_State.ctl" = cluster{"State":enum16{"Initialize", "SetDefaultConfig", "Close", "Quit", "Identify", "MoveAbs", "MoveAbs_all", "MoveRel", "MoveRel_all", "STOP", "Origin/Home", "WaitStop", "QueryStatus", "UpdateXPos", "UpdateAll", "SetVelocity", "SetAcceleration", "ClearErr", "LogMessage", "MotorEnable(1)", "EnableAxis", "JoyStick", "GetVelocity", "GetAcceleration", "SendCmd", "SetSoftLimits", "Beep", "_SettingReturn", "SoftReset"}, "Params.":variant}
  T75 = typedef "Signal.ctl" = cluster{"Command":T76, "Params":variant}
  T76 = typedef "ProcessStates.ctl" = enum16{"Initialize", "Normal", "Display", "Write2Buffer", "CalcMzArray", "StartSave", "StopSave", "ConfigChanged", "EndOfLine", "SetFilterParams", "SetGraphsEnable", "SetAcquisitionParams", "ChangeDisplayIncrement", "ChangeRepRate", "SetWriterRef", "Quit", "StartOfLine"}
  T77 = typedef "BinaryHeader.ctl" = cluster{"Start Position":dbl[], "StepWidth":dbl[], "Dimension":i32[], "SpecLength":i32}
  T78 = typedef "BeamProfiling_Params.ctl" = cluster{"File Header":T77, "w_fit_init.":dbl[], "z0_fit_init.":dbl[], "LowSpeed":dbl, "HighSpeed":dbl, "x/y?":bool, "IncidentAngle":dbl}
  T79 = typedef "Imaging_Params.ctl" = cluster{"File Header":T77, "ScanSpeed":dbl, "HighSpeed":dbl, "SampleRate":T12, "Rep.Rate (Hz)":dbl, "TrigDelay":dbl, "mzCali":dbl[], "KeepStill(ms)":u32, "SaveRaw":bool}
  T80 = cluster{"MotionStageRefs":refnum<queue>, "Axis#":i32, "Delay(ps)":dbl, "ZeroDelay_Offset":dbl}
  T81 = typedef "SRS_DG535_Lib.lvlib/DG535_States.ctl" = cluster{"State":enum16{"Initialize", "Set Trigger", "Set Output", "Set Delay", "Manl_Trig", "Run", "Stop", "Close", "Quit"}, "Para.":variant}
  T82 = typedef "EPM2K_Status.ctl" = cluster{"State":enum16{"Initialize", "Idle/Update", "Configure", "Read", "Close", "Quit"}, "Parameter":dbl}
  T83 = typedef "BNC_States.ctl" = cluster{"State":enum16{"Initialize", "Set System", "Set C-Input", "Set C-Mode", "Set C-Output", "Set C-Enable", "Manl_Trig", "Run", "Stop", "Query C Number", "Close", "Quit"}, "Para.":variant}
  T84 = typedef "DAQmx_Status.ctl" = cluster{"State":enum16{"Initialize", "Idle", "Update", "Close", "Quit"}, "Para.":variant}
  T85 = typedef "Micos_uic.lvlib/Micos_State.ctl" = cluster{"State":enum16{"Initialize", "SetDefaultConfig", "Close", "Quit", "Identify", "MoveAbs", "MoveAbs_all", "MoveRel", "MoveRel_all", "STOP", "Origin/Home", "WaitStop", "QueryStatus", "UpdateXPos", "UpdateAll", "SetVelocity", "SetAcceleration", "ClearErr", "LogMessage", "MotorEnable(1)", "EnableAxis", "JoyStick", "GetVelocity", "GetAcceleration", "SendCmd", "SetSoftLimits", "Beep", "_SettingReturn", "SoftReset"}, "Params.":variant}
  T86 = cluster{"Rep.Rate":dbl, "Sys Ext Mode":enum16{"Disabled", "Triggered", "Gated", "Triggered & Gated"}, "Mode":enum16{"Normal", "Single Shot", "Duty Cycle", "Burst"}}
  T87 = typedef "IMAQdx.ctl" = refnum<k21>
  T88 = cluster{"Coupling":u16, "Differential Input":bool, "Direct-to-ADC":bool, "Range":u32, "Impedance":u32, "DC Offset":i32, "Filter":i32}[]
  T89 = cluster{"Coupling":u16, "Differential Input":bool, "Direct-to-ADC":bool, "Range":u32, "Impedance":u32, "DC Offset":i32, "Filter":i32}
  T90 = cluster{"axes total":u32, "buttons total":u32, "pov total":u32, "device name":string}[]
  T91 = enum16{"MouseClick", "MouseDoubleClick", "MouseRightClick", "SetCalibration", "AutoCalibration"}
  T92 = typedef "NI_Matrix.lvlib/RealMatrix.ctl" = dbl[][]
  T93 = typedef "ImageConvPara.ctl" = cluster{"Start Position":dbl[], "StepWidth":dbl[], "Dimension":i32[], "ScanSpeed":dbl}
  T94 = typedef "ImageConvPara_3d.ctl" = cluster{"Start Position":dbl[], "StepWidth":dbl[], "Dimension":i32[], "MeanderSpeed":dbl}
  T95 = typedef "DepthProfilingParams.ctl" = cluster{"SamplingPos.":cluster{"x":dbl, "y":dbl, "z":dbl}[][], "z-depth (ms)":u32, "Idle(ms)":u32, "HighSpeed":dbl, "RepRate (Hz)":dbl}
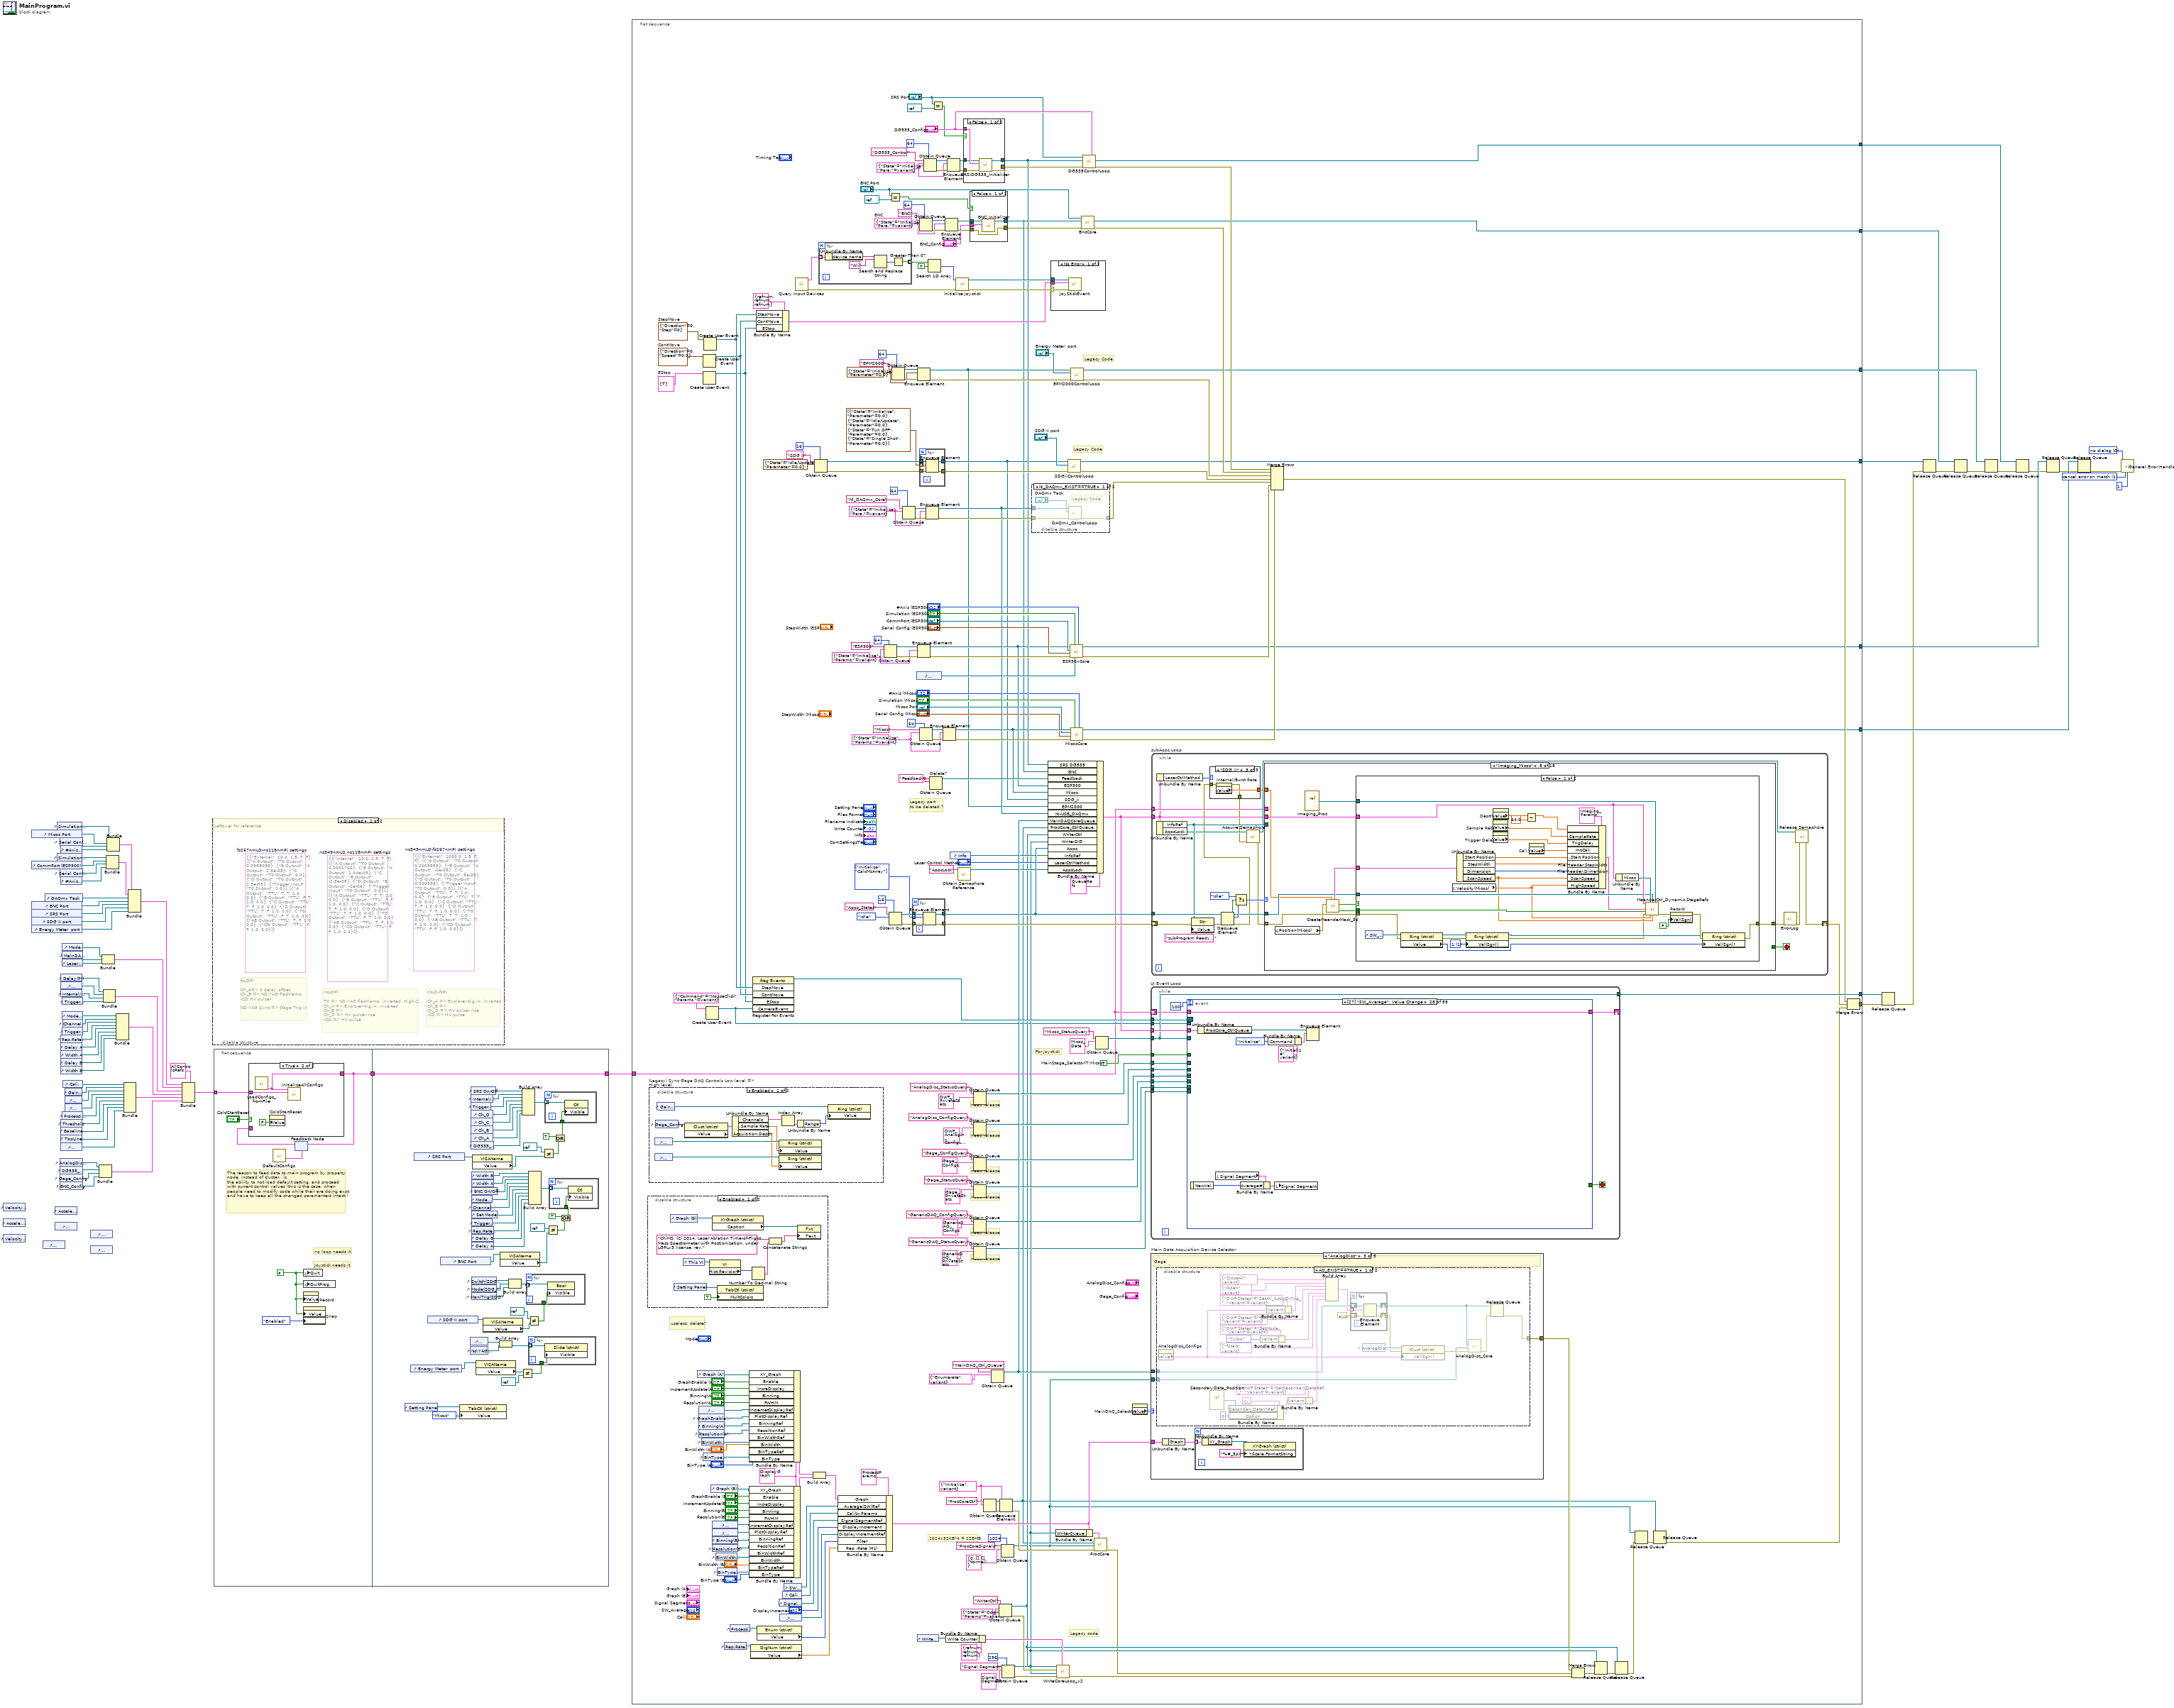
[diagram p0: block diagram]
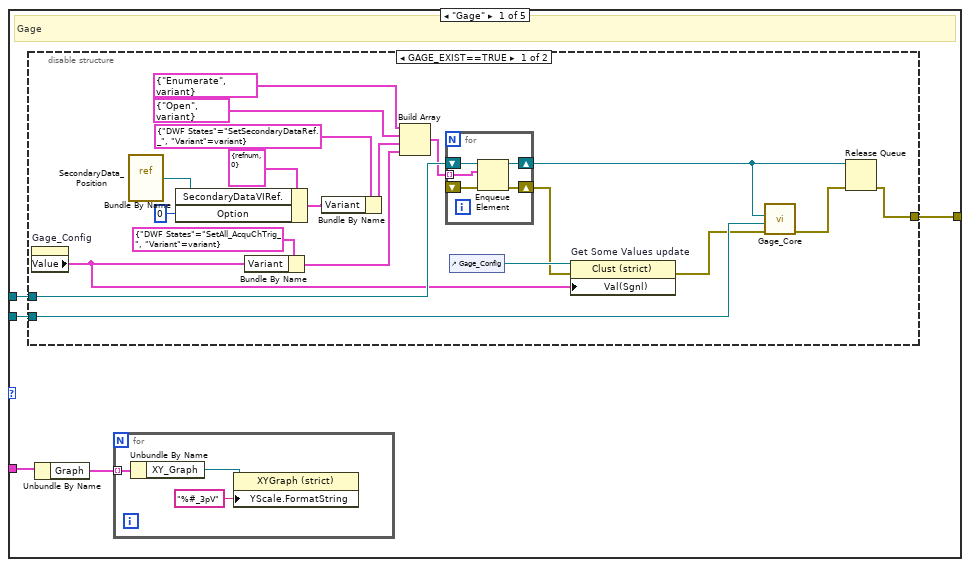
[diagram p8: hidden frame]
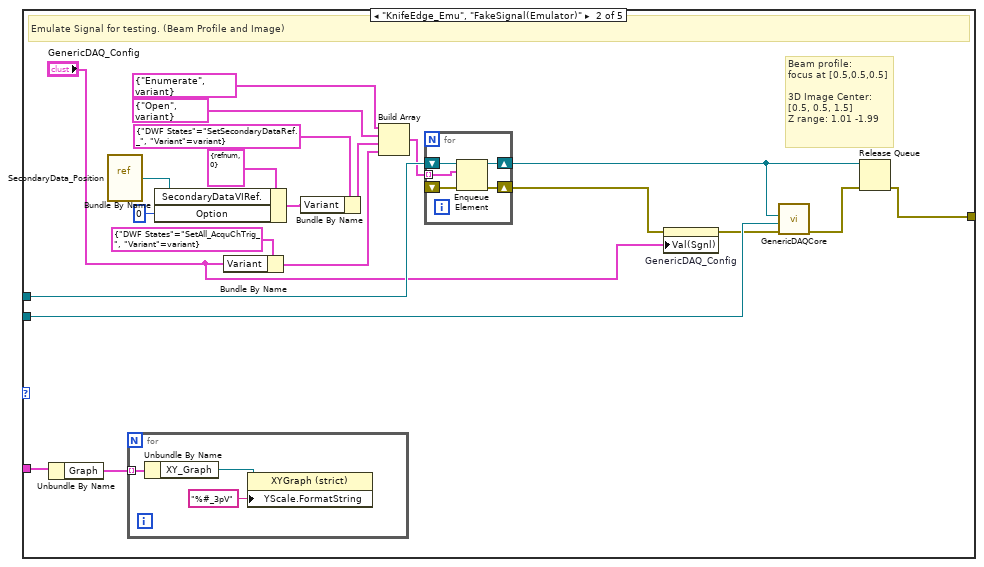
[diagram p10: hidden frame]
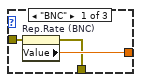
[diagram p14: hidden frame]
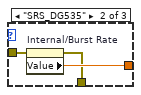
[diagram p15: hidden frame]
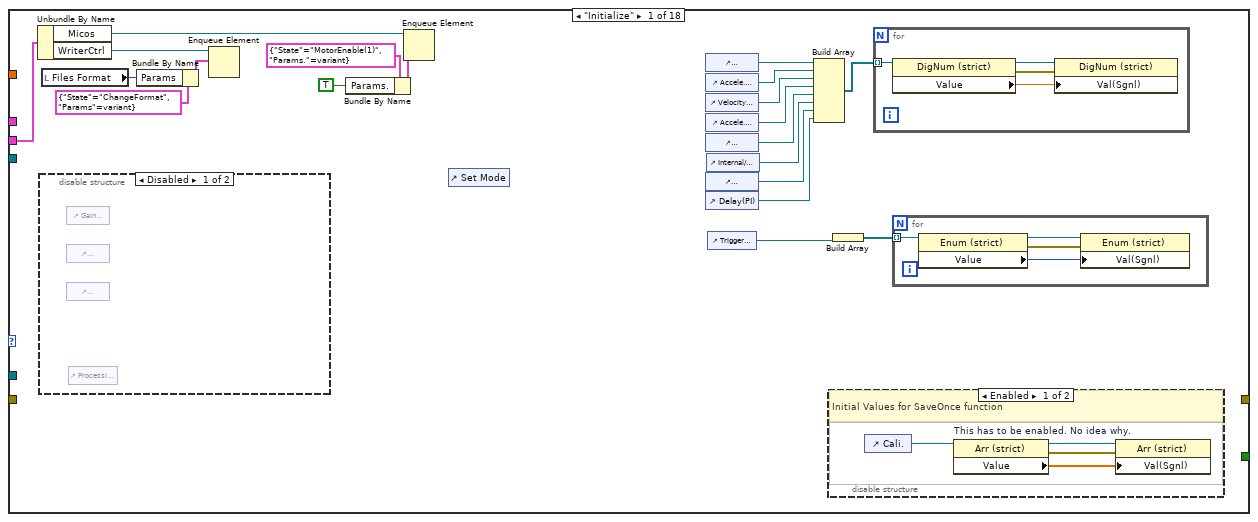
[diagram p16: hidden frame]
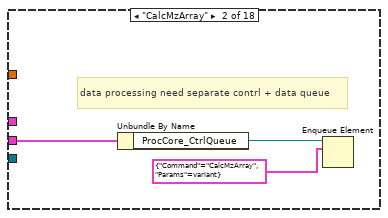
[diagram p19: hidden frame]
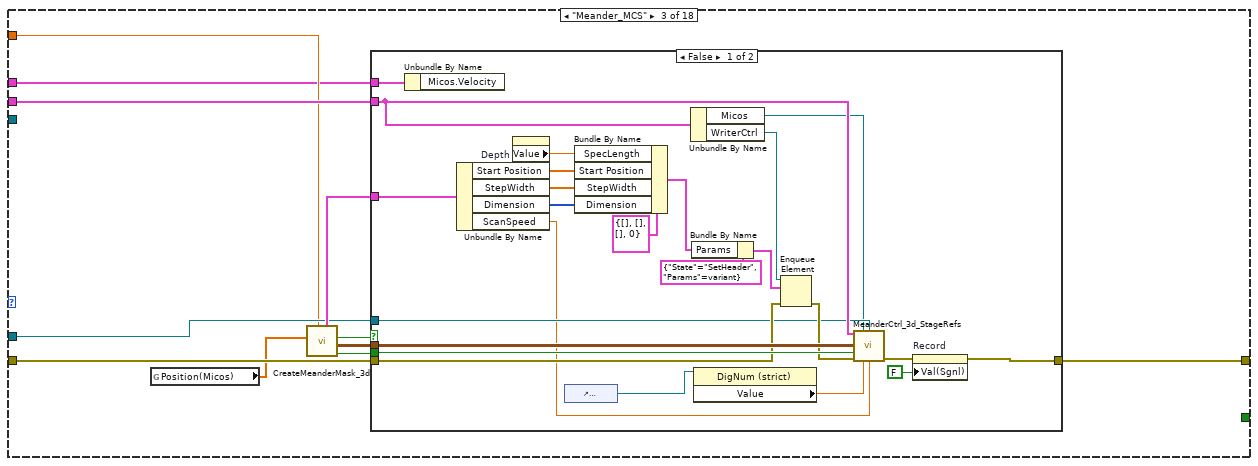
[diagram p20: hidden frame]
diagram:
  w56 = 1 items=["no exception", "cancel error on match", "set error on match"] ("[exception action] (none:0)")
  w57 = T39 0 items=["no dialog", "OK message", "continue or stop message", "OK message + warnings", "continue/stop + warnings"] ("type of dialog (OK msg:1)")
  n1 = control-ref of="Velocity (ESP) #3"() -> ()  [unwired: 1 out]
  n2 = control-ref of="Accele. (ESP)"() -> ()  [unwired: 1 out]
  n3 = control-ref of="Velocity (ESP)"() -> ()  [unwired: 1 out]
  n4 = control-ref of="Micos Port"() -> (w49:refnum<vi>)
  n5 = control-ref of="CommPort (ESP300)"() -> (w52:refnum<vi>)
  n6 = control-ref of="BNC Port"() -> (w45:refnum<vi>)
  n7 = control-ref of="SRS Port"() -> (w44:refnum<vi>)
  n8 = control-ref of="SDG II port"() -> (w42:refnum<vi>)
  n9 = control-ref of="Energy Meter  port"() -> (w43:refnum<vi>)
  n10 = control-ref of="ZeroDelayPos"() -> ()  [unwired: 1 out]
  n11 = control-ref of="DAQmx Task"() -> (w6:refnum<vi>)
  n12 = control-ref of="Accele.(Micos)"() -> ()  [unwired: 1 out]
  n13 = control-ref of="Velocity(Micos)"() -> ()  [unwired: 1 out]
  n14 = control-ref of="Simulation (Micos)"() -> (w47:refnum<vi>)
  n15 = control-ref of="Simulation (ESP300)"() -> (w53:refnum<vi>)
  n16 = control-ref of="Serial Config (Micos)"() -> (w48:refnum<vi>)
  n17 = control-ref of="Serial Config (ESP300)"() -> (w51:refnum<vi>)
  n18 = control-ref of="AnalogDisc_Configs"() -> (w37:refnum<vi>)
  n19 = control-ref of="DG535_Configs"() -> (w38:refnum<vi>)
  n20 = control-ref of="Gage_Config"() -> (w39:refnum<vi>)
  n21 = control-ref of="BNC_Config"() -> (w3:refnum<vi>)
  n22 = control-ref of="#Axis (Micos)"() -> (w46:refnum<vi>)
  n23 = control-ref of="#Axis (ESP300)"() -> (w50:refnum<vi>)
  n24 = control-ref of="Delay(PI)"() -> (w33:refnum<vi>)
  n25 = control-ref of="Delay(LDI-Rej.)"() -> (w32:refnum<vi>)
  n26 = control-ref of="Internal/Burst Rate"() -> (w31:refnum<vi>)
  n27 = control-ref of="Rep.Rate (BNC)"() -> (w27:refnum<vi>)
  n28 = control-ref of="Delay A"() -> (w26:refnum<vi>)
  n29 = control-ref of="Width A"() -> (w25:refnum<vi>)
  n30 = control-ref of="Delay B"() -> (w24:refnum<vi>)
  n31 = control-ref of="Width B"() -> (w23:refnum<vi>)
  n32 = control-ref of="Threshold"() -> (w17:refnum<vi>)
  n33 = control-ref of="Baseline"() -> (w16:refnum<vi>)
  n34 = control-ref of="TopLine"() -> (w15:refnum<vi>)
  n35 = control-ref of="ZeroOffsetCorrection"() -> (w14:refnum<vi>)
  n36 = control-ref of="Mode"() -> (w34:refnum<vi>)
  n37 = control-ref of="MainDAQ_Selector"() -> (w36:refnum<vi>)
  n38 = control-ref of="Laser Control Method"() -> (w35:refnum<vi>)
  n39 = control-ref of="Trigger Mode (SRS)"() -> (w30:refnum<vi>)
  n40 = control-ref of="Mode (BNC)"() -> (w29:refnum<vi>)
  n41 = control-ref of="Trigger Mode (BNC)"() -> (w28:refnum<vi>)
  n42 = control-ref of="Processing Mode"() -> (w18:refnum<vi>)
  n43 = control-ref of="Channels Enable Status"() -> (w1:refnum<vi>)
  n44 = control-ref of="Cali."() -> (w22:refnum<vi>)
  n45 = control-ref of="Gain (Voltage Range)"() -> (w21:refnum<vi>)
  n46 = control-ref of="Spectrum Length"() -> (w20:refnum<vi>)
  n47 = control-ref of="SampleRate"() -> (w19:refnum<vi>)
  n48 = control-ref of="YAGEnergyCoeff."() -> ()  [unwired: 1 out]
  n49 = control-ref of="fsEnergyCoeff."() -> ()  [unwired: 1 out]
  n50 = Bundle("AnalogDisc_Configs"=w37, "DG535_Configs"=w38, "Gage_Config"=w39, "BNC_Config"=w3) -> (w9:T40)  [unwired: 1 in]
  n51 = Bundle("Mode"=w34, "MainDAQ_Selector"=w36, "Laser Control Method"=w35) -> (w13:T41)  [unwired: 1 in]
  n52 = Bundle("Delay(PI)"=w33, "Delay(LDI-Rej.)"=w32, "Internal/Burst Rate"=w31, "Trigger Mode (SRS)"=w30) -> (w12:T42)  [unwired: 1 in]
  n53 = Bundle("Simulation (ESP300)"=w53, "CommPort (ESP300)"=w52, "Serial Config (ESP300)"=w51, "#Axis (ESP300)"=w50) -> (w41:T43)  [unwired: 1 in]
  n54 = Bundle("Simulation (Micos)"=w47, "Micos Port"=w49, "Serial Config (Micos)"=w48, "#Axis (Micos)"=w46) -> (w40:T44)  [unwired: 1 in]
  n55 = Bundle("Mode (BNC)"=w29, "Channels Enable Status"=w1, "Trigger Mode (BNC)"=w28, "Rep.Rate (BNC)"=w27, "Delay A"=w26, "Width A"=w25, "Delay B"=w24, "Width B"=w23) -> (w11:T45)  [unwired: 1 in]
  n56 = Bundle("Cali."=w22, "Gain (Voltage Range)"=w21, "Spectrum Length"=w20, "SampleRate"=w19, "Processing Mode"=w18, "Threshold"=w17, "Baseline"=w16, "TopLine"=w15, "ZeroOffsetCorrection"=w14) -> (w10:T46)  [unwired: 1 in]
  n57 = Bundle(w40, w41, "DAQmx Task"=w6, "BNC Port"=w45, "SRS Port"=w44, "SDG II port"=w42, "Energy Meter  port"=w43) -> (w8:T47)  [unwired: 1 in]
  n58 = Bundle(cluster=T38 {"Communication"={"Micos"={"Simulation (Micos)"=refnum, "Micos Port"=refnum, "Serial Config (Micos)"=refnum, "#Axis (Micos)"=refnum}, "ESP300"={"Simulation (ESP300)"=refnum, "CommPort (ESP300)"=refnum, "Serial Config (ESP300)"=refnum, "#Axis (ESP300)"=refnum}, "DAQmx Task"=refnum, "BNC Port"=refnum, "SRS Port"=refnum, "SDG_II port"=refnum, "EnergyMeter port"=refnum}, "Method"={"Mode"=refnum, "MainDAQ_Selector"=refnum, "LaserCtrlMethod"=refnum}, "DG535"={"Delay(PI)"=refnum, "Delay(LDI-Rej.)"=refnum, "Internal/Burst Rate"=refnum, "Trigger Mode (SRS)"=refnum}, "BNC"={"Mode (BNC)"=refnum, "Channels Enable Status"=refnum, "Trigger Mode (BNC)"=refnum, "Rep.Rate (BNC)"=refnum, "Delay A"=refnum, "Width A"=refnum, "Delay B"=refnum, "Width B"=refnum}, "Expt"={"Cali."=refnum, "Gain (Voltage Range)"=refnum, "Spectrum Length"=refnum, "SampleRate"=refnum, "Processing Mode"=refnum, "Threshold"=refnum, "Baseline"=refnum, "TopLine"=refnum, "ZeroOffsetCorrection"=refnum}, "LowLevel"={"AnalogDisc_Configs"=refnum, "DG535_Configs"=refnum, "Gage_Config"=refnum, "BNC_Config"=refnum}}, "Communication"=w8, "Method"=w13, "DG535"=w12, "BNC"=w11, "Expt"=w10, "LowLevel"=w9) -> (w2:T38)
  n59 = disable-structure shown="Disabled" {
    frame Disabled {
      (unwired) T48 {"Trigger"={"Trigger Mode"=enum."Internal", "Internal/Burst Rate"=10.0, "External  Level"=1.5, "Impedance"=TRUE, "Slope"=FALSE}, "Delays"=[{"Channel"=enum."A Output", "Sync To"=enum."T0 Output", "Delay"=0.0001766}, {"Channel"=enum."B Output", "Sync To"=enum."A Output", "Delay"=1.44e-05}, {"Channel"=enum."C Output", "Sync To"=enum."B Output", "Delay"=-2.5e-05}, {"Channel"=enum."D Output", "Sync To"=enum."B Output", "Delay"=-2e-06}, {"Channel"=enum."Trigger Input", "Sync To"=enum."T0 Output", "Delay"=0.0}], "Output"=[{"Channel"=enum."A Output", "Level"=enum."TTL", "Load"=TRUE, "Polarity"=TRUE, "Amplitude"=1.0, "Offset"=0.0}, {"Channel"=enum."B Output", "Level"=enum."TTL", "Load"=FALSE, "Polarity"=FALSE, "Amplitude"=1.0, "Offset"=0.0}, {"Channel"=enum."C Output", "Level"=enum."TTL", "Load"=TRUE, "Polarity"=FALSE, "Amplitude"=1.0, "Offset"=0.0}, {"Channel"=enum."D Output", "Level"=enum."TTL", "Load"=TRUE, "Polarity"=FALSE, "Amplitude"=1.0, "Offset"=0.0}, {"Channel"=enum."T0 Output", "Level"=enum."TTL", "Load"=FALSE, "Polarity"=TRUE, "Amplitude"=1.0, "Offset"=0.0}, {"Channel"=enum."AB Output", "Level"=enum."TTL", "Load"=TRUE, "Polarity"=FALSE, "Amplitude"=1.0, "Offset"=0.0}, {"Channel"=enum."CD Output", "Level"=enum."TTL", "Load"=FALSE, "Polarity"=FALSE, "Amplitude"=1.0, "Offset"=0.0}]}  # ns349nmLD,ns118nmPI settings
      (unwired) T48 {"Trigger"={"Trigger Mode"=enum."External", "Internal/Burst Rate"=10.0, "External  Level"=1.5, "Impedance"=TRUE, "Slope"=FALSE}, "Delays"=[{"Channel"=enum."A Output", "Sync To"=enum."T0 Output", "Delay"=0.0998095}, {"Channel"=enum."B Output", "Sync To"=enum."A Output", "Delay"=2.5e-05}, {"Channel"=enum."C Output", "Sync To"=enum."T0 Output", "Delay"=0.0}, {"Channel"=enum."D Output", "Sync To"=enum."T0 Output", "Delay"=2.3e-05}, {"Channel"=enum."Trigger Input", "Sync To"=enum."T0 Output", "Delay"=0.0}], "Output"=[{"Channel"=enum."A Output", "Level"=enum."TTL", "Load"=TRUE, "Polarity"=TRUE, "Amplitude"=1.0, "Offset"=0.0}, {"Channel"=enum."B Output", "Level"=enum."TTL", "Load"=FALSE, "Polarity"=TRUE, "Amplitude"=1.0, "Offset"=0.0}, {"Channel"=enum."C Output", "Level"=enum."TTL", "Load"=TRUE, "Polarity"=FALSE, "Amplitude"=1.0, "Offset"=0.0}, {"Channel"=enum."D Output", "Level"=enum."TTL", "Load"=TRUE, "Polarity"=FALSE, "Amplitude"=1.0, "Offset"=0.0}, {"Channel"=enum."T0 Output", "Level"=enum."TTL", "Load"=FALSE, "Polarity"=TRUE, "Amplitude"=1.0, "Offset"=0.0}, {"Channel"=enum."AB Output", "Level"=enum."TTL", "Load"=TRUE, "Polarity"=FALSE, "Amplitude"=1.0, "Offset"=0.0}, {"Channel"=enum."CD Output", "Level"=enum."TTL", "Load"=FALSE, "Polarity"=FALSE, "Amplitude"=1.0, "Offset"=0.0}]}  # fs267nmLD-ns118nmPI settings
      (unwired) T48 {"Trigger"={"Trigger Mode"=enum."External", "Internal/Burst Rate"=1000.0, "External  Level"=1.5, "Impedance"=TRUE, "Slope"=FALSE}, "Delays"=[{"Channel"=enum."A Output", "Sync To"=enum."T0 Output", "Delay"=0.0009859}, {"Channel"=enum."B Output", "Sync To"=enum."A Output", "Delay"=-2e-05}, {"Channel"=enum."C Output", "Sync To"=enum."T0 Output", "Delay"=5e-05}, {"Channel"=enum."D Output", "Sync To"=enum."T0 Output", "Delay"=0.000998}, {"Channel"=enum."Trigger Input", "Sync To"=enum."T0 Output", "Delay"=0.0}], "Output"=[{"Channel"=enum."A Output", "Level"=enum."TTL", "Load"=TRUE, "Polarity"=TRUE, "Amplitude"=1.0, "Offset"=0.0}, {"Channel"=enum."B Output", "Level"=enum."TTL", "Load"=TRUE, "Polarity"=TRUE, "Amplitude"=1.0, "Offset"=0.0}, {"Channel"=enum."C Output", "Level"=enum."TTL", "Load"=TRUE, "Polarity"=FALSE, "Amplitude"=1.0, "Offset"=0.0}, {"Channel"=enum."D Output", "Level"=enum."TTL", "Load"=TRUE, "Polarity"=FALSE, "Amplitude"=1.0, "Offset"=0.0}, {"Channel"=enum."T0 Output", "Level"=enum."TTL", "Load"=TRUE, "Polarity"=TRUE, "Amplitude"=1.0, "Offset"=0.0}, {"Channel"=enum."AB Output", "Level"=enum."TTL", "Load"=TRUE, "Polarity"=FALSE, "Amplitude"=1.0, "Offset"=0.0}, {"Channel"=enum."CD Output", "Level"=enum."TTL", "Load"=FALSE, "Polarity"=FALSE, "Amplitude"=1.0, "Offset"=0.0}]}  # ns349nmLD-fs267nmPI settings
      # "nsLD-fsPI\n\nCh_A => Explorer trig in, inverted\nCh_B => \nCh_D => HV pulser rise\n-CD => HV pulse"
      # "nsLDPI\n\nT0 => ND:YAG flashlamp, inverted, High-Z\nCh_A => Explorer trig in, inverted\nCh_B => \nCh_D => HV pulser rise\n-CD => HV pulse"
      # "fsLDPI\n\nCh_A=> 0 delay offset\nCh_B => ND:YAG flashlamp\n-CD HV pulser\n\nND:YAG Sync => Gage Trig in"
      # "Leftover for reference"
    }
    frame Enabled {
    }
  }
  n60 = flat-sequence {
    tunnel: [w75] -> w5
    tunnel: w2 -> [w72]
    tunnel: [w92] -> w4
    tunnel: w5 -> [w92]
    frame #0 {
      w74 = FALSE
      # "no loop needs it"
      # "Joystick needs it"
      # "The reason to feed data to main program by property \nnode, instead of cluster,  is\nthe ability to not load default setting, and proceed \nwith current control values (this is the case, when \npeople need to modify code while their are doing expt\nand have to keep all the changed paramenters intact.)"
      n61 = call "DefaultConfigs.vi"() -> ("Configuration 2"=w76:T50)  [unwired: 11 in]
      n62 = feedback #1(w76) -> (w77:T50)
      n63 = case shown="True" "ColdStartReset" {
        tunnel: w72 -> [w80 w83]
        tunnel: [w81 w82] -> w75
        tunnel: w77 -> [w79 _]
        frame False {
          n64 = call "BuildConfigsFromFrontPanel.vi"("AllControlsRefs"=w80, "InstruConfig"=w79) -> ("InstruConfig out"=w81:T50)  [unwired: 9 in]
        }
        frame True {
          n65 = call "LoadConfigs_fromFile.vi"() -> ("Configuration"=w82:T50)  [unwired: 11 in]
          n66 = property on="ColdStartReset" class="Bool (strict)"("Value"=FALSE ("ResetSettings")) -> ()  [unwired: 2 in, 2 out]
          n67 = call "InitializeAllConfigs.vi"("AllControlsRefs"=w83, "InstruConfig"=w82) -> ()  [unwired: 10 in]
        }
      }
      n68 = feedback-in #1(w75) -> ()
      n69 = local write "Quit"(w74) -> ()
      n70 = global write "QuitProg.vi" "QuitProg."(w74) -> ()
      n71 = property on="Record" class="Bool (strict)"("Value"=w74) -> ()  [unwired: 2 in, 2 out]
      n72 = property on="Snap" class="Bool (strict)"("Value"=w74, "DisabledEnum"=T49."Enabled" ("Disabled")) -> ()  [unwired: 2 in, 2 out]
    }
    frame #1 {
      n73 = control-ref of="Setting Panel"() -> (w86:refnum<vi>)
      n74 = control-ref of="Energy Meter  port"() -> (w93:refnum<vi>)
      n75 = control-ref of="SRS Port"() -> (w100:refnum<vi>)
      n76 = control-ref of="SDG II port"() -> (w95:refnum<vi>)
      n77 = control-ref of="BNC Port"() -> (w97:refnum<vi>)
      n78 = property class="TabCtl (strict)"(reference=w86, "Value"=T5."Micos") -> ()  [unwired: 1 in, 2 out]
      n79 = control-ref of="LaserEnergy"() -> (w121:refnum<vi>)
      n80 = control-ref of="Nd:YAG Energy"() -> (w122:refnum<vi>)
      n81 = control-ref of="SRS On/Off"() -> (w134:refnum<vi>)
      n82 = control-ref of="Internal/Burst Rate"() -> (w133:refnum<vi>)
      n83 = control-ref of="Trigger Mode (SRS)"() -> (w132:refnum<vi>)
      n84 = control-ref of="Ch_D"() -> (w131:refnum<vi>)
      n85 = control-ref of="Ch_C"() -> (w130:refnum<vi>)
      n86 = control-ref of="Ch_B"() -> (w129:refnum<vi>)
      n87 = control-ref of="Ch_A"() -> (w128:refnum<vi>)
      n88 = control-ref of="DG535_Configs"() -> (w124:refnum<vi>)
      n89 = control-ref of="Switch(SDG_II)"() -> (w113:refnum<vi>)
      n90 = control-ref of="Mode(SDG_II)"() -> (w114:refnum<vi>)
      n91 = control-ref of="ManlTrig(SDG)"() -> (w115:refnum<vi>)
      n92 = control-ref of="Width B"() -> (w101:refnum<vi>)
      n93 = control-ref of="Width A"() -> (w102:refnum<vi>)
      n94 = control-ref of="BNC On/Off"() -> (w103:refnum<vi>)
      n95 = control-ref of="Mode (BNC)"() -> (w104:refnum<vi>)
      n96 = control-ref of="Channels Enable Status"() -> (w105:refnum<vi>)
      n97 = control-ref of="Set Mode"() -> (w106:refnum<vi>)
      n98 = control-ref of="Trigger Mode (BNC)"() -> (w107:refnum<vi>)
      n99 = control-ref of="Rep.Rate (BNC)"() -> (w108:refnum<vi>)
      n100 = control-ref of="Delay B"() -> (w109:refnum<vi>)
      n101 = control-ref of="Delay A"() -> (w110:refnum<vi>)
      n102 = property class="VISAName"(reference=w100) -> ("Value"=w99:refnum<visa-resource-name>)  [unwired: 1 in, 2 out]
      n103 = property class="VISAName"(reference=w93) -> ("Value"=w94:refnum<visa-resource-name>)  [unwired: 1 in, 2 out]
      n104 = property class="VISAName"(reference=w95) -> ("Value"=w96:refnum<visa-resource-name>)  [unwired: 1 in, 2 out]
      n105 = Build Array(w121, w122) -> (w123:refnum<vi>[])
      n106 = property class="VISAName"(reference=w97) -> ("Value"=w98:refnum<visa-resource-name>)  [unwired: 1 in, 2 out]
      n107 = Build Array(w113, w114, w115) -> (w118:refnum<vi>[])
      n108 = Not Equal?(x=w94, y=refnum<visa-resource-name> refnum ("BNC Port")) -> (x != y?=w119:bool)
      n109 = Build Array(w134, w133, w132, w131, w130, w129, w128, w124) -> (w125:refnum<vi>[])
      n110 = Not Equal?(x=refnum<visa-resource-name> refnum ("BNC Port"), y=w96) -> (x != y?=w116:bool)
      n111 = for {
        tunnel: w118 -> [w138] mode=indexing
        tunnel: w116 -> [w137]
        n112 = property class="Bool"(reference=w138, "Visible"=w137) -> ()  [unwired: 1 in, 2 out]
      }
      n113 = Build Array(w101, w102, w103, w104, w105, w106, w107, w108, w109, w110) -> (w111:refnum<vi>[])
      n114 = for {
        tunnel: w123 -> [w136] mode=indexing
        tunnel: w119 -> [w135]
        n115 = property class="Slide (strict)"(reference=w136, "Visible"=w135) -> ()  [unwired: 1 in, 2 out]
      }
      n116 = Not Equal?(x=refnum<visa-resource-name> refnum ("BNC Port"), y=w99) -> (x != y?=w127:bool)
      n117 = Not Equal?(x=refnum<visa-resource-name> refnum ("BNC Port"), y=w98) -> (x != y?=w91:bool)
      n118 = Or(x=TRUE, y=w127) -> (x .or. y?=w88:bool)
      n119 = for {
        tunnel: w125 -> [w142] mode=indexing
        tunnel: w88 -> [w141]
        n120 = property class="Ctl"(reference=w142, "Visible"=w141) -> ()  [unwired: 1 in, 2 out]
      }
      n121 = Or(x=TRUE, y=w91) -> (x .or. y?=w90:bool)
      n122 = for {
        tunnel: w111 -> [w140] mode=indexing
        tunnel: w90 -> [w139]
        n123 = property class="Ctl"(reference=w140, "Visible"=w139) -> ()  [unwired: 1 in, 2 out]
      }
    }
  }
  n124 = flat-sequence {
    tunnel: [w234] -> w71
    tunnel: [w221] -> w70
    tunnel: [w219] -> w68
    tunnel: [w217] -> w67
    tunnel: [w216] -> w66
    tunnel: [w215] -> w64
    tunnel: [w214] -> w62
    tunnel: [w213] -> w61
    tunnel: w4 -> [w158]
    frame #0 {
      w157 = T75 {"Command"=enum."Initialize", "Params"=variant} ("element")
      w198 = cluster{"EStop":bool} {"EStop"=TRUE}  # EStop
      w203 = cluster{"Direction":i32, "Speed":dbl} {"Direction"=0, "Speed"=0.0}  # ContMove
      w204 = cluster{"Direction":i32, "Step":i32} {"Direction"=0, "Step"=0}  # StepMove
      w205 = TRUE  # MainStage_Selector(T:Micos)
      w280 = T67 {"XY_Graph"=refnum, "Enable"=FALSE, "IncreDisplay"=FALSE, "Binning"=FALSE, "IncremetDisplayRef"=refnum, "PlotDisplayRef"=refnum, "BinningRef"=refnum, "FWHM"=FALSE, "ResoltionRef"=refnum, "BinWidthRef"=refnum, "BinWidth"=0.0, "BinTypeRef"=refnum, "BinType"=enum."ByTime"} ("Graph")
      w243 = T74 {"State"=enum."Initialize", "Params."=variant} ("Cluster")
      w248 = T81 {"State"=enum."Initialize", "Para."=variant} ("element")
      w256 = T83 {"State"=enum."Initialize", "Para."=variant}  # BNC
      w285 = T74 {"State"=enum."Initialize", "Params."=variant} ("Cluster")
      w323 = T82 {"State"=enum."Initialize", "Parameter"=0.0} ("Idle")
      w328 = T84 {"State"=enum."Initialize", "Para."=variant} ("Micos States")
      w350 = "Feedback"
      w358 = T71[] [enum."Initialize", enum."CalcMzArray"] items=["Initialize", "Idle", "CalcMzArray", "Meander_SGL_MCS", "Meander_MCS", "CleanSurface", "Meander_Npt", "Meander_SGL_Npt", "KnifeEdgeExpt", "KnifeEdgeExpt_Npt", "Imaging_Micos", "Imaging_ESP", "DepthProfiling", "Set_2PulseDelay", "DelayScan", "PeakSearch", "ExportOrigin", "Save Settings", "Load Settings", "Save as Default", "Load Default", "EnergyCalibration", "Quit", "Interrupted_Stop", "Quit_SubProgram", "StepMove_Joystick", "ContMove_Joystick", "Stop_Joystick", "Check_AppsLock", "Return_Status", "DepthProfile_RT", "UpdateInstruStates", "InstruOptimizer_static", "InstruOptimizer_dynamic", "DepthProfiling(3D)"]
      # "need release"
      # "need release"
      # "useless, delete?"
      # "For joystick"
      # "Legacy part\nto be deleted ?"
      # "Legacy Code"
      # "Legacy Code"
      # "Legacy code"
      # "need release"
      # "need release"
      # "need release"
      # "need release"
      # "1024x32KB*4 = 128MB"
      n125 = disable-structure shown="Enabled" {
        frame Enabled {
          n126 = control-ref of="Graph (B)"() -> (w371:refnum<vi>)
          n127 = control-ref of="Setting Panel"() -> (w378:refnum<vi>)
          n128 = control-ref of="This VI"() -> (w376:refnum<vi>)
          n129 = property class="VI"(reference=w376) -> ("Hist.Revision"=w373:u32)  [unwired: 1 in, 2 out]
          n130 = property class="XYGraph (strict)"(reference=w371) -> ("Caption"=w370:refnum<vi>)  [unwired: 1 in, 2 out]
          n131 = property class="TabCtl (strict)"(reference=w378, "MultColors"=TRUE ("Allow Multiple Colors")) -> ()  [unwired: 1 in, 2 out]
          n132 = Number To Decimal String(number=w373) -> (decimal integer string=w372:string)  [unwired: 1 in]
          n133 = Concatenate Strings("ChiMS, (C) 2014, Laser Ablation Time-of-Flight Mass Spectrometer with Postionization, under LGPLv3 license, rev." ("string"), w372) -> (w375:string)
          n134 = property class="Txt"(reference=w370, "Text"=w375) -> ()  [unwired: 1 in, 2 out]
        }
        frame Disabled {
        }
      }
      n135 = disable-structure "(Legacy) Sync Gage DAQ Controls Low level =>  High level" shown="Enabled" {
        frame Enabled {
          n136 = control-ref of="SampleRate"() -> (w386:refnum<vi>)
          n137 = control-ref of="Spectrum Length"() -> (w388:refnum<vi>)
          n138 = control-ref of="Gage_Config"() -> (w384:refnum<vi>)
          n139 = control-ref of="Gain (Voltage Range)"() -> (w387:refnum<vi>)
          n140 = property class="Clust (strict)"(reference=w384) -> ("Value"=w385:T19)  [unwired: 1 in, 2 out]
          n141 = Unbundle By Name(w385) -> ("Channels"=w381:T88, "Acquisition.Sample Rate"=w383:dbl, "Acquisition.Depth"=w382:dbl)
          n142 = property class="Ring (strict)"(reference=w386, "Value"=w383) -> ()  [unwired: 1 in, 2 out]
          n143 = property class="Ring (strict)"(reference=w388, "Value"=w382) -> ()  [unwired: 1 in, 2 out]
          n144 = Index Array(array=w381) -> (element=w380:T89)  [unwired: 1 in]
          n145 = Unbundle By Name(w380) -> ("Range"=w379:u32)
          n146 = property class="Ring (strict)"(reference=w387, "Value"=w379) -> ()  [unwired: 1 in, 2 out]
        }
        frame Disabled {
        }
      }
      n147 = control-ref of="Graph (A)"() -> (w314:refnum<vi>)
      n148 = control-ref of="IncrementUpdate(A)"() -> (w306:refnum<vi>)
      n149 = control-ref of="GraphEnable (A)"() -> (w305:refnum<vi>)
      n150 = control-ref of="Binning(A)"() -> (w304:refnum<vi>)
      n151 = control-ref of="Resolution(A)"() -> (w291:refnum<vi>)
      n152 = control-ref of="BinWidth (A)"() -> (w284:refnum<vi>)
      n153 = Create User Event(user event datatype=w203) -> (user event=w201:refnum<user-event>)  [unwired: 1 in, 1 out]
      n154 = Create User Event(user event datatype=w198) -> (user event=w197:refnum<user-event>)  [unwired: 1 in, 1 out]
      n155 = control-ref of="BinType (A)"() -> (w282:refnum<vi>)
      n156 = Create User Event(user event datatype=w204) -> (user event=w202:refnum<user-event>)  [unwired: 1 in, 1 out]
      n157 = Create User Event(user event datatype=T54 {"Command"=enum."MouseClick", "Params."=variant} ("CameraEvent")) -> (user event=w159:refnum<user-event>)  [unwired: 1 in, 1 out]
      n158 = control-ref of="Graph (B)"() -> (w313:refnum<vi>)
      n159 = control-ref of="IncrementUpdate(B)"() -> (w300:refnum<vi>)
      n160 = control-ref of="GraphEnable(B)"() -> (w299:refnum<vi>)
      n161 = control-ref of="Binning(B)"() -> (w298:refnum<vi>)
      n162 = control-ref of="Resolution(B)"() -> (w290:refnum<vi>)
      n163 = control-ref of="BinWidth (B)"() -> (w279:refnum<vi>)
      n164 = control-ref of="BinType (B)"() -> (w277:refnum<vi>)
      n165 = control-ref of="Rep.Rate (BNC)"() -> (w266:refnum<vi>)
      n166 = control-ref of="Processing Mode"() -> (w275:refnum<vi>)
      n167 = Bundle By Name(cluster=w280, "XY_Graph"=w314, "Enable"="GraphEnable (A)", "IncreDisplay"="IncrementUpdate(A)", "Binning"="Binning(A)", "FWHM"="Resolution(A)", "IncremetDisplayRef"=w306, "PlotDisplayRef"=w305, "BinningRef"=w304, "ResoltionRef"=w291, "BinWidthRef"=w284, "BinWidth"="BinWidth (A)", "BinTypeRef"=w282, "BinType"="BinType (A)") -> (w312:T67)
      n168 = Bundle By Name(cluster=w280, "XY_Graph"=w313, "Enable"="GraphEnable (B)", "IncreDisplay"="IncrementUpdate(B)", "Binning"="Binning(B)", "FWHM"="Resolution(B)", "IncremetDisplayRef"=w300, "PlotDisplayRef"=w299, "BinningRef"=w298, "ResoltionRef"=w290, "BinWidthRef"=w279, "BinWidth"="BinWidth (B)", "BinTypeRef"=w277, "BinType"="BinType (B)") -> (w311:T67)
      n169 = property class="DigNum (strict)"(reference=w266) -> ("Value"=w265:dbl)  [unwired: 1 in, 2 out]
      n170 = register-events(w202, w201, w197, w159) -> (reference out=w294:refnum<event-registration>)  [unwired: 2 in, 1 out]
      n171 = Bundle By Name(cluster=T53 {"StepMove"=refnum, "ContMove"=refnum, "EStop"=refnum}, "StepMove"=w202, "ContMove"=w201, "EStop"=w197) -> (w200:T53)
      n172 = property class="Enum (strict)"(reference=w275) -> ("Value"=w274:T4)  [unwired: 1 in, 2 out]
      n173 = control-ref of="Signal Segment"() -> (w295:refnum<vi>)
      n174 = control-ref of="DisplayIncrement"() -> (w264:refnum<vi>)
      n175 = control-ref of="Cali."() -> (w296:refnum<vi>)
      n176 = control-ref of="SW Average"() -> (w297:refnum<vi>)
      n177 = call <vilib>:"Query Input Devices.vi"() -> ("error out"=w322:errorcluster, "joystick info"=w193:T90)  [unwired: 8 in, 2 out]
      n178 = Build Array(w312, w311) -> (w310:T67[])
      n179 = Obtain Queue(max queue size (-1, unlimited)=16, name (unnamed)="SDG II", element data type=T70 {"State"=enum."Idle/Update", "Parameter"=0.0} ("Cluster")) -> (queue out=w346:refnum<queue>, error out=w347:errorcluster)  [unwired: 2 in, 1 out]
      n180 = for {
        tunnel: w193 -> [w402] mode=indexing
        tunnel: [w398] -> w196 mode=indexing
        n181 = Unbundle By Name(w402) -> ("device name"=w401:string)
        n182 = Search and Replace String(input string=w401, search string="Wii") -> (number of replacements=w399:i32)  [unwired: 6 in, 3 out]
        n183 = Greater Than 0?(x=w399) -> (x > 0?=w398:bool)
      }
      n184 = Bundle By Name(cluster=T65 {"DisplayIncrement"=0, "DisplayIncrementRef"=refnum, "Rep .Rate (Hz)"=0.0, "Save"=FALSE, "SW_Average"=0, "Filter"=enum."None", "FilterParams"=variant, "DAQParams"={"TrigDelay"=0.0, "Offset"=0, "Resolution"=0, "Range (mV)"=0, "Sample Rate"=0.0, "Depth"=0.0, "Segments"=0}, "Graph"=[], "CmdParams."=variant, "Average(SW)Ref"=refnum, "Calibr.Params"=refnum, "SignalSegmentRef"=refnum, "WriterQueue"=refnum}, "Graph"=w310, "Average(SW)Ref"=w297, "Calibr.Params"=w296, "SignalSegmentRef"=w295, "DisplayIncrement"="DisplayIncrement", "DisplayIncrementRef"=w264, "Filter"=w274, "Rep .Rate (Hz)"=w265) -> (w262:T65)
      n185 = Obtain Queue(max queue size (-1, unlimited)=64, name (unnamed)="ESP300", element data type=w285) -> (queue out=w348:refnum<queue>, error out=w349:errorcluster)  [unwired: 2 in, 1 out]
      n186 = Obtain Queue(max queue size (-1, unlimited)=16, name (unnamed)="Apps_States", element data type=States-AToF."Idle" ("Ring")) -> (queue out=w362:refnum<queue>, error out=w361:errorcluster)  [unwired: 2 in, 1 out]
      n187 = Equal?(x="BNC Port", y=refnum<visa-resource-name> refnum ("SRS Port")) -> (x = y?=w152:bool)
      n188 = Obtain Queue(max queue size (-1, unlimited)=64, name (unnamed)="EPM2000", element data type=w323) -> (queue out=w325:refnum<queue>, error out=w324:errorcluster)  [unwired: 2 in, 1 out]
      n189 = Obtain Queue(max queue size (-1, unlimited)=64, name (unnamed)="NI_DAQmx_Core", element data type=w328) -> (queue out=w329:refnum<queue>, error out=w331:errorcluster)  [unwired: 2 in, 1 out]
      n190 = for {
        tunnel: w362 -> [w1084]
        tunnel: w361 -> [w1083]
        tunnel: [w1082] -> w269
        tunnel: [w1081] -> w351
        tunnel: w358 -> [w1080] mode=indexing
        n191 = Enqueue Element(queue=w1084, element=w1080, error in (no error)=w1083) -> (queue out=w1082:refnum<queue>, error out=w1081:errorcluster)  [unwired: 1 in, 1 out]
      }
      n192 = control-ref of="MotorDisabled(ESP)"() -> (w260:refnum<vi>)
      n193 = control-ref of="Write Counter"() -> (w336:refnum<vi>)
      n194 = Enqueue Element(queue=w325, element=w323, error in (no error)=w324) -> (queue out=w218:refnum<queue>, error out=w327:errorcluster)  [unwired: 1 in, 1 out]
      n195 = Enqueue Element(queue=w348, element=w285, error in (no error)=w349) -> (queue out=w244:refnum<queue>, error out=w340:errorcluster)  [unwired: 1 in, 1 out]
      n196 = Obtain Queue(max queue size (-1, unlimited)=64, name (unnamed)="BNC", element data type=w256) -> (queue out=w258:refnum<queue>, error out=w259:errorcluster)  [unwired: 2 in, 1 out]
      n197 = Obtain Queue(max queue size (-1, unlimited)=64, name (unnamed)="Micos", element data type=w243) -> (queue out=w359:refnum<queue>, error out=w360:errorcluster)  [unwired: 2 in, 1 out]
      n198 = for {
        tunnel: [w515] -> w341
        tunnel: w347 -> [w514]
        tunnel: w346 -> [w513]
        tunnel: [w512] -> w220
        tunnel: T70[] [{"State"=enum."Initialize", "Parameter"=0.0}, {"State"=enum."Idle/Update", "Parameter"=0.0}, {"State"=enum."Tun OFF", "Parameter"=0.0}, {"State"=enum."Single Shot", "Parameter"=0.0}] -> [w511] mode=indexing
        n199 = Enqueue Element(queue=w513, element=w511, error in (no error)=w514) -> (queue out=w512:refnum<queue>, error out=w515:errorcluster)  [unwired: 1 in, 1 out]
      }
      n200 = Obtain Queue(max queue size (-1, unlimited)=64, name (unnamed)="DG535_Control", element data type=w248) -> (queue out=w247:refnum<queue>, error out=w250:errorcluster)  [unwired: 2 in, 1 out]
      n201 = Enqueue Element(queue=w329, element=w328, error in (no error)=w331) -> (queue out=w271:refnum<queue>, error out=w330:errorcluster)  [unwired: 1 in, 1 out]
      n202 = Search 1D Array(1D array=w196, element=TRUE) -> (index of element=w194:i32)  [unwired: 1 in]
      n203 = Obtain Queue "Delete?"(name (unnamed)=w350, element data type=w350) -> (queue out=w272:refnum<queue>)  [unwired: 3 in, 2 out]
      n204 = Equal?(x="SRS Port", y=refnum<visa-resource-name> refnum ("SRS Port")) -> (x = y?=w231:bool)
      n205 = Enqueue Element(queue=w359, element=w243, error in (no error)=w360) -> (queue out=w242:refnum<queue>, error out=w339:errorcluster)  [unwired: 1 in, 1 out]
      n206 = Enqueue Element(queue=w258, element=w256, error in (no error)=w259) -> (queue out=w156:refnum<queue>, error out=w150:errorcluster)  [unwired: 1 in, 1 out]
      n207 = Bundle By Name(cluster=T69 {"Write Counter"=refnum, "Segment Counter"=refnum, "Writer error out"=refnum} ("Controls ref."), "Write Counter"=w336) -> (w337:T69)
      n208 = Enqueue Element(queue=w247, element=w248, error in (no error)=w250) -> (queue out=w246:refnum<queue>, error out=w249:errorcluster)  [unwired: 1 in, 1 out]
      n209 = control-ref of="Info"() -> (w268:refnum<vi>)
      n210 = call <vilib>:"Initialize Joystick.vi"("error in (no error)"=w322, "device index"=w194) -> ("error out"=w192:errorcluster, "device ID"=w321:refnum<k1>)  [unwired: 8 in]
      n211 = call <vilib>:"Obtain Semaphore Reference.vi"("name (unnamed)"="AppsLock") -> ("semaphore"=w206:T63)  [unwired: 4 in, 2 out]
      n212 = case shown="False" w231 {
        tunnel: [w407 w408] -> w253
        tunnel: [w406 w409] -> w252
        tunnel: "DG535_Configs" -> [w405 _]
        tunnel: w249 -> [w404 w409]
        tunnel: w246 -> [w403 w408]
        frame False {
          n213 = call "SRS-DG535_Initializer.vi"("error in (no error)"=w404, "DG535_Configs"=w405, "Queue in"=w403) -> ("error out"=w406:errorcluster, "Queue out"=w407:refnum<queue>)  [unwired: 7 in]
        }
        frame True {
        }
      }
      n214 = case shown="False" w152 {
        tunnel: w156 -> [w392 w394]
        tunnel: [w391 w394] -> w155
        tunnel: [w390 w393] -> w151
        tunnel: w150 -> [w390 w393]
        tunnel: "BNC_Config" -> [w389 _]
        frame False {
          n215 = call "BNC_Initializer.vi"("BNC_Config"=w389, "BNC Control Queue in"=w392) -> ("BNC Ctrl queue out"=w391:refnum<queue>)  [unwired: 9 in]
        }
        frame True {
        }
      }
      n216 = Obtain Queue(name (unnamed)="AnalogDisc_StatusQuery", element data type=T57 {"Handle_DWF"=0, "Model"="", "SN"="", "TrigRate(Hz)"=0.0, "TrigCount"=0, "Mode"=enum."Normal", "STS"=enum."stsRdy", "SecondaryDataParams."={"SecondaryDataVIRef."=refnum, "Option"=0}} ("PrivateStats(Live)")) -> (queue out=w185:refnum<queue>)  [unwired: 3 in, 2 out]
      n217 = Obtain Queue(name (unnamed)="AnalogDisc_ConfigQuery", element data type=T20 {"Acqusition"={"Freq(Hz,SampleRate)"=10000000.0, "BufferSize"=8192, "Mode"=enum."Single", "RecordLength(s)"=0.0}, "Channels"=[{"Range(V)"=5.0, "Offset(V)"=0.0, "Filter"=enum."Decimate", "Enable"=TRUE}], "Trigger"={"TriggerSource"=enum."None", "Timeout(s)"=0.0, "Holdoff(s)"=1e-06, "Position(s)"=0.0}, "AnalogTrigger"={"Channel"=0, "Polarity"=enum."Rising", "Type"=enum."Pulse", "Level(V)"=0.0, "Filter"=enum."Decimate", "Hysterisis(V)"=0.0}} ("AnalogDisc_Configs 2")) -> (queue out=w183:refnum<queue>)  [unwired: 3 in, 2 out]
      n218 = Obtain Queue(name (unnamed)="Gage_ConfigQuery", element data type=T19 {"Acquisition"={"Sample Rate"=100000000.0, "Mode"=1, "Start (0)"=8192.0, "Depth"=8192.0, "Segment Size"=100.0, "Trigger Delay"=0.0, "Trigger Timeout"=0.0, "Trigger Holdoff"=0.0, "Clock mode"=enum."Internal", "Segment"=0}, "Channels"=[{"Coupling"=0, "Differential Input"=FALSE, "Direct-to-ADC"=FALSE, "Range"=2000, "Impedance"=50, "DC Offset"=0, "Filter"=0}, {"Coupling"=0, "Differential Input"=FALSE, "Direct-to-ADC"=FALSE, "Range"=2000, "Impedance"=50, "DC Offset"=0, "Filter"=0}], "Trigger"={"Slope"=0, "Level"=0, "Source"=0, "External Range"=2000, "External Coupling"=0, "External"=TRUE, "Disable"=FALSE, "External Impedance"=0}, "Mode(Gage)"=enum."Continuous"} ("Gage_Config")) -> (queue out=w180:refnum<queue>)  [unwired: 3 in, 2 out]
      n219 = Obtain Queue(name (unnamed)="Gage_StatusQuery", element data type=T55 {"Model"="", "TrigRate(Hz)"=0.0, "TrigCount"=0, "Mode(Gage)"=enum."Normal", "Handle"={"Handle"=0, "Sample size"=0, "Resolution"=0, "Offset"=0, "Channels"=0, "Boards"=0}, "DAQ_Status"=enum."Done", "SecondaryDataVIRef"=refnum, "Option(SecondaryDataVI)"=0, "cSegment"=0, "TSArray"=[], "Adj.SegmenttSize"=0.0} ("PrivateStats(Live)")) -> (queue out=w177:refnum<queue>)  [unwired: 3 in, 2 out]
      n220 = Obtain Queue(name (unnamed)="GenericDAQ_ConfigQuery", element data type=T14 {"Acquisition"={"Sample Rate"=1000000000.0, "Mode"=0, "Start (0)"=0.0, "Depth"=1024.0, "Segment"=1}, "Channels"=[{"Range"=1, "DC Offset"=0}], "Mode(Gage)"=enum."Continuous"} ("GenericDAQ_Config")) -> (queue out=w146:refnum<queue>)  [unwired: 3 in, 2 out]
      n221 = Obtain Queue(name (unnamed)="GenericDAQ_StatusQuery", element data type=T51 {"Model"="", "TrigRate(Hz)"=0.0, "TrigCount"=0, "Mode"=enum."Normal", "DAQ_Status"=enum."Done", "SecondaryDataVIRef"=refnum, "Option(SecondaryDataVI)"=0, "cSegment"=0} ("PrivateStats(Live)")) -> (queue out=w144:refnum<queue>)  [unwired: 3 in, 2 out]
      n222 = Obtain Queue(name (unnamed)="ProcCoreCtrl", element data type=w157) -> (queue out=w188:refnum<queue>, error out=w187:errorcluster)  [unwired: 3 in, 1 out]
      n223 = Obtain Queue(name (unnamed)="MainDAQ_Ctrl_Queue", element data type=T60 {"DWF States"=enum."Enumerate", "Variant"=variant}) -> (queue out=w270:refnum<queue>)  [unwired: 3 in, 2 out]
      n224 = Obtain Queue(name (unnamed)="WriterCtrl", element data type=T68 {"State"=enum."Open", "Params"=variant} ("Writer_State")) -> (queue out=w173:refnum<queue>, error out=w332:errorcluster)  [unwired: 3 in, 1 out]
      n225 = Enqueue Element(queue=w188, element=w157) -> (queue out=w163:refnum<queue>)  [unwired: 2 in, 2 out]
      n226 = Obtain Queue(max queue size (-1, unlimited)=1024, name (unnamed)="ProcCoreSignals", element data type=T59 {"tickcount"=0, "Signal"=[], "SecondaryData"=[], "Flag"=enum."Normal"} ("Signal_Typedef")) -> (queue out=w162:refnum<queue>)  [unwired: 2 in, 2 out]
      n227 = Obtain Queue(max queue size (-1, unlimited)=256, name (unnamed)="Signal Segment", element data type=T3 {"SampleRate"=0.0, "TrigDelay"=0.0, "SpecLength"=0.0, "DAQ_Range"=0.0, "Average#"=0, "Position"=[], "Spectrum"=[], "Calibr."=[], "Pressure"=0.0, "Desp_LaserEnergy"=0.0, "PI_LaserEnergy"=0.0, "Voltages Table"=[], "ProcMode"=enum."None", "Threshold"=0.0, "Comment"="", "TickCount"=0.0, "Time Stamp"=timestamp(0 s since 1904-01-01)} ("Signal Segment")) -> (queue out=w171:refnum<queue>, error out=w335:errorcluster)  [unwired: 2 in, 1 out]
      n228 = disable-structure shown="NI_DAQmx_EXIST==TRUE" {
        disable-tunnel: w330 -> [w368 w369]
        disable-tunnel: w271 -> [w367 _]
        disable-tunnel: [w366 w369] -> w227
        frame condition #0 {
          # "Legacy Code"
          n229 = call "DAQmx_ControlLoop.vi"("error in"=w368, "DAQmx Task Name"="DAQmx Task", "queue out"=w367) -> ("error out"=w366:errorcluster)  [unwired: 8 in]
        }
        frame condition #1 (active) {
        }
      }
      n230 = Bundle By Name(cluster=T62 {"LaserCtrlMethod"=enum."SRS_DG535", "Apps"=refnum, "MainDAQCoreQueue"=refnum, "Micos"=refnum, "ESP300"=refnum, "SMC100"=refnum, "SRS DG535"=refnum, "BNC"=refnum, "SDG_ii"=refnum, "NI-USB_DAQmx"=refnum, "ProcCore_CtrlQueue"=refnum, "WriterCtrl"=refnum, "WriterSIG"=refnum, "Feedback"=refnum, "EPM2000"=refnum, "InfoRef"=refnum, "AppsLock"=refnum, "ProcCore_SignalQueue"=refnum}, "SRS DG535"=w253, "BNC"=w155, "Feedback"=w272, "ESP300"=w244, "Micos"=w242, "SDG_ii"=w220, "EPM2000"=w218, "NI-USB_DAQmx"=w271, "MainDAQCoreQueue"=w270, "ProcCore_CtrlQueue"=w163, "WriterCtrl"=w173, "WriterSIG"=w171, "Apps"=w269, "InfoRef"=w268, "LaserCtrlMethod"="Laser Control Method", "AppsLock"=w206) -> (w263:T62)
      n231 = case shown="No Error" w192 {
        selector: w192 -> [w395 _]
        tunnel: w321 -> [w397 _]
        tunnel: w200 -> [w396 _]
        frame No Error {
          n232 = call "JoyStickEvent.vi"("error in"=w395, "UserEvent_Handle"=w396, "device ID"=w397) -> ()  [unwired: 9 in]
        }
        frame Error {
        }
      }
      n233 = Bundle By Name(cluster=w262, "WriterQueue"=w171) -> (w245:T65)
      n234 = call "WriteCoreLoop_v2.vi"("Controls ref."=w337, "data error in"=w335, "data queue in"=w171, 10:"control queue in"=w332, 11:"control queue in"=w173) -> ("error out"=w168:errorcluster)  [unwired: 6 in]
      n235 = call "SDGiiControlLoop.vi"("queue error in"=w341, "VISA resource"="SDG II port", "queue in"=w220) -> ("error out"=w226:errorcluster, "queue out"=w219:refnum<queue>)  [unwired: 7 in]
      n236 = call <instrlib>:"ESP30xCore.vi"("NumOfAxis"="#Axis (ESP300)", "MotorDisabled"=w260, "Simulation"="Simulation (ESP300)", "error in"=w340, "Serial Configuration"="Serial Config (ESP300)", "CommPort"="CommPort (ESP300)", "ControlQueue in"=w244) -> ("error out"=w228:errorcluster, "queue out"=w213:refnum<queue>)  [unwired: 3 in]
      n237 = call <instrlib>:"MicosCore.vi"("NumOfAxis"="#Axis (Micos)", "Simulation"="Simulation (Micos)", "error in"=w339, "Serial Configuration"="Serial Config (Micos)", "CommPort"="Micos Port", "ControlQueue in"=w242) -> ("error out"=w229:errorcluster, "queue out"=w214:refnum<queue>)  [unwired: 4 in]
      n238 = call "EPM2000ControlLoop.vi"("queue error in"=w327, "VISA resource"="Energy Meter  port", "Control queue in"=w218) -> ("error out"=w225:errorcluster, "queue out"=w217:refnum<queue>)  [unwired: 7 in]
      n239 = call "BncCore.vi"("error in"=w151, "queue in"=w155, "VISA resource"="BNC Port") -> ("error out"=w224:errorcluster, "queue out"=w216:refnum<queue>)  [unwired: 7 in]
      n240 = call <instrlib>:"DG535ControlLoop.vi"("Settings"="DG535_Configs", "error in"=w252, "queue in"=w253, "VISA resource"="SRS Port") -> ("error out"=w223:errorcluster, "queue out"=w215:refnum<queue>)  [unwired: 6 in]
      n241 = call "ProcCore.vi"("ProcessParams"=w245, "error in"=w187, "SignalBuffer in"=w162, "CtrlQueue in"=w163) -> ("error out"=w169:errorcluster)  [unwired: 7 in]
      n242 = Obtain Queue(name (unnamed)="Micos_StatusQuery", element data type=T64 {"Position"=[], "Velocity"=[], "Acceleration"=[], "Moving"=FALSE, "Simulation"=FALSE, "tickcount_mov"=0, "tickcount_pos"=0, "NumOfAxis"=0, "Initialized"=FALSE, "CommPort"="", "Range"=[], "Serial Configuration"={"Baud Rate"=0, "Parity"=0, "Data Bits"=0, "Stop Bits"=0, "Flow Control"=0}, "MotorDisabled"=refnum}) -> (queue out=w236:refnum<queue>)  [unwired: 3 in, 2 out]
      n243 = property on="MainDAQ_Selector" class="Enum (strict)"() -> ("Value"=w176:T16)  [unwired: 2 in, 2 out]
      n244 = while "UI Event Loop" {
        tunnel: w294 -> [w1097]
        tunnel: w263 -> [w1096]
        tunnel: w236 -> [w1095]
        tunnel: [w1095] -> w234
        tunnel: w205 -> [w1094]
        tunnel: w185 -> [w1093]
        tunnel: w183 -> [w1092]
        tunnel: w180 -> [w1091]
        tunnel: w177 -> [w1090]
        tunnel: w159 -> [w1088]
        shift-right: [w1087] -> _
        shift-left: w158 -> [w1089]
        tunnel: w146 -> [w1086]
        tunnel: w144 -> [w1085]
        stop <- w1099 stop-if-true
        n245 = event shown="[27] \"SW_Average\": Value Change" {
          selector: w1097 -> [_ _ _ _ _ _ _ _ _ _ _ _ _ _ _ _ _ _ _ _ _ _ _ _ _ _ _ _ _ _ _ _ _ _ _ _ _ _ _ _ _ _ _ _ _ _ _ _ _ _ _ _ _ _ _ _ _ _ _]
          dyn-events: _ -> [_ _ _ _ _ _ _ _ _ _ _ _ _ _ _ _ _ _ _ _ _ _ _ _ _ _ _ _ _ _ _ _ _ _ _ _ _ _ _ _ _ _ _ _ _ _ _ _ _ _ _ _ _ _ _ _ _ _ _]
          timeout: 100 -> [_ _ _ _ _ _ _ _ _ _ _ _ _ _ _ _ _ _ _ _ _ _ _ _ _ _ _ _ _ _ _ _ _ _ _ _ _ _ _ _ _ _ _ _ _ _ _ _ _ _ _ _ _ _ _ _ _ _ _]
          tunnel: [_ TRUE ("status") w1175 _ _ _ _ _ _ _ _ _ _ _ _ _ _ _ _ _ _ _ _ _ _ _ _ _ _ _ _ _ _ _ _ _ _ _ _ _ _ _ _ _ _ _ _ _ _ _ _ _ _ _ _ _ _ _ _] -> w1099
          tunnel: w1096 -> [w1125 w1169 w1176 w1280 w1283 w1292 w1311 w1324 w1331 w1339 w1346 w1388 w1423 w1460 w1484 w1500 w1520 w1534 w1542 w1558 _ _ w1589 w1600 w1628 w1664 w1701 w1709 w1720 w1726 w1736 w1742 w1746 w1760 w1789 w1797 _ w1812 w1828 _ w1845 w1868 w1894 w1924 _ w2008 w2019 w2026 w2063 w2106 _ _ _ _ _ _ _ _ _]
          tunnel: w1095 -> [w1116 _ _ _ _ _ _ _ _ _ _ _ _ _ _ _ _ _ _ _ _ _ _ _ _ _ _ _ _ _ _ _ _ _ _ _ _ _ _ _ _ _ _ _ _ _ _ _ _ _ _ _ _ _ _ _ _ _ _]
          tunnel: w1094 -> [_ _ _ _ _ _ _ _ _ _ w1347 w1389 w1425 _ _ _ _ _ _ _ _ _ _ _ _ _ _ _ _ _ _ _ _ _ _ _ _ _ _ _ _ _ _ _ _ _ _ _ _ _ _ _ _ _ _ _ _ _ _]
          tunnel: w1093 -> [w1111 _ _ _ _ _ _ _ _ _ _ _ _ _ _ _ _ _ _ _ _ _ _ _ _ _ _ _ _ _ _ _ _ _ _ _ _ _ _ _ _ _ _ _ _ _ _ _ _ _ _ _ _ _ _ _ _ _ _]
          tunnel: w1092 -> [_ _ _ _ _ _ _ _ _ _ _ _ _ _ _ _ _ _ _ _ _ _ _ _ w1623 _ _ _ _ _ _ _ _ _ _ _ _ _ _ _ _ _ _ _ _ _ _ _ _ _ _ _ _ _ _ _ _ _ _]
          tunnel: w1091 -> [_ _ _ _ _ _ _ _ _ _ _ _ _ _ _ _ _ _ _ _ _ _ _ _ _ w1649 _ _ _ _ _ _ _ _ _ _ _ _ _ _ _ _ _ _ _ _ _ _ _ _ _ _ _ _ _ _ _ _ _]
          tunnel: w1090 -> [w1112 _ _ _ _ _ _ _ _ _ _ _ _ _ _ _ _ _ _ _ _ _ _ _ _ _ _ _ _ _ _ _ _ _ _ _ _ _ _ _ _ _ _ _ _ _ _ _ _ _ _ _ _ _ _ _ _ _ _]
          tunnel: w1089 -> [w1109 w1168 w1174 w1261 w1281 w1289 w1309 w1322 w1326 w1333 w1341 w1381 w1421 w1441 w1478 w1498 w1518 w1527 w1535 w1548 w1565 w1571 w1581 w1592 w1604 w1634 w1674 w1707 w1718 w1724 w1733 w1740 w1744 w1758 w1787 w1795 w1803 w1810 w1818 w1836 w1839 w1864 w1889 w1915 w1950 w2001 w2012 w2023 w2060 w2103 w2111 w2129 w2131 w2138 w2161 w2171 w2196 w2231 w2244]
          tunnel: w1088 -> [_ _ _ _ _ _ _ _ _ _ _ _ _ _ _ _ _ _ _ _ _ _ _ _ _ _ _ _ _ _ _ _ _ _ _ _ _ _ _ _ _ _ _ _ _ _ _ _ _ _ _ _ _ _ _ _ _ _ w2245]
          tunnel: [w1109 w1168 w1174 w1261 w1281 w1288 w1308 w1322 w1326 w1333 w1341 w1381 w1421 w1441 w1478 w1498 w1518 w1527 w1535 w1548 w1565 w1571 w1580 w1591 w1603 w1633 w1674 w1707 w1717 w1724 w1732 w1740 w1744 w1757 w1787 w1795 w1803 w1810 w1818 w1836 w1839 w1863 w1890 w1914 w1947 w2000 w2012 w2023 w2060 w2103 w2111 w2129 w2131 w2138 w2161 w2171 w2196 w2231 w2244] -> w1087
          tunnel: w1086 -> [_ _ _ _ _ _ _ _ _ _ _ _ _ _ _ _ _ _ _ _ _ _ _ _ _ _ w1671 _ _ _ _ _ _ _ _ _ _ _ _ _ _ _ _ _ _ _ _ _ _ _ _ _ _ _ _ _ _ _ _]
          tunnel: w1085 -> [w1100 _ _ _ _ _ _ _ _ _ _ _ _ _ _ _ _ _ _ _ _ _ _ _ _ _ _ _ _ _ _ _ _ _ _ _ _ _ _ _ _ _ _ _ _ _ _ _ _ _ _ _ _ _ _ _ _ _ _]
          event Timeout {
            n246 = event-data() -> ()  [unwired: 1 in, 1 out]
            n247 = Unbundle By Name(w1125) -> ("MainDAQCoreQueue"=w1115:refnum<queue>, "Micos"=w1124:refnum<queue>)
            n248 = Bundle By Name(cluster=T85 {"State"=enum."QueryStatus", "Params."=variant} ("element"), "Params."=w1116) -> (w1127:T85)
            n249 = Enqueue Element "Set return ref."(queue=w1124, element=w1127) -> (error out=w1129:errorcluster)  [unwired: 2 in, 2 out]
            n250 = case "Refresh Trigger Rate (Hz)" shown="\"KnifeEdge_Emu\", \"FakeSignal(Emulator)\"" "MainDAQ_Selector" {
              tunnel: w1115 -> [_ w1146 w1154 w1162]
              tunnel: [0 ("TrigCount") w1140 w1148 w1156] -> w1114
              tunnel: w1112 -> [_ _ w1147 _]
              tunnel: w1111 -> [_ w1139 _ _]
              tunnel: w1100 -> [_ _ _ w1155]
              frame "None", Default {
              }
              frame "AnalogDisc" {
                n251 = Bundle By Name(cluster=T60 {"DWF States"=enum."GetStat_", "Variant"=variant} ("element"), "Variant"=w1139) -> (w1144:T60)
                n252 = Enqueue Element "Set Return Ref."(queue=w1146, element=w1144) -> (error out=w1142:errorcluster)  [unwired: 2 in, 2 out]
                n253 = Dequeue Element(queue=w1139, timeout in ms (-1)=1000, error in (no error)=w1142) -> (element=w1141:T57)  [unwired: 3 out]
                n254 = Unbundle By Name(w1141) -> ("TrigCount"=w1140:i32)
              }
              frame "Gage" {
                n255 = Bundle By Name(cluster=T60 {"DWF States"=enum."GetStat_", "Variant"=variant} ("element"), "Variant"=w1147) -> (w1152:T60)
                n256 = Enqueue Element "Set Return Ref."(queue=w1154, element=w1152) -> (error out=w1150:errorcluster)  [unwired: 2 in, 2 out]
                n257 = Dequeue Element(queue=w1147, timeout in ms (-1)=1000, error in (no error)=w1150) -> (element=w1149:T55)  [unwired: 3 out]
                n258 = Unbundle By Name(w1149) -> ("TrigCount"=w1148:i32)
              }
              frame "KnifeEdge_Emu", "FakeSignal(Emulator)" {
                n259 = Bundle By Name(cluster=T60 {"DWF States"=enum."GetStat_", "Variant"=variant} ("element"), "Variant"=w1155) -> (w1160:T60)
                n260 = Enqueue Element "Set Return Ref."(queue=w1162, element=w1160) -> (error out=w1158:errorcluster)  [unwired: 2 in, 2 out]
                n261 = Dequeue Element(queue=w1155, timeout in ms (-1)=1000, error in (no error)=w1158) -> (element=w1157:T51)  [unwired: 3 out]
                n262 = Unbundle By Name(w1157) -> ("TrigCount"=w1156:i32)
              }
            }
            n263 = global read "MiscParams.vi" "IonLaserEnergy"() -> (w1132:dbl)
            n264 = Dequeue Element(queue=w1116, timeout in ms (-1)=1000, error in (no error)=w1129) -> (element=w1123:T64)  [unwired: 3 out]
            n265 = global read "MiscParams.vi" "DspLaserEnergy"() -> (w1135:dbl)
            n266 = Unbundle By Name(w1123) -> ("Position"=→"Position(Micos)":dbl[], "Velocity"=w1122:dbl[], "Acceleration"=w1121:dbl[], "Moving"=→"Moving (Micos)":bool)  [unwired: 1 out]
            n267 = Multiply(x="fsEnergyCoeff.", y=w1135) -> (x*y=w1130:dbl)
            "LaserEnergy" <- w1130
            n268 = Multiply(x="YAGEnergyCoeff.", y=w1132) -> (x*y=w1131:dbl)
            "Nd:YAG Energy" <- w1131
            n269 = Index Array(array=w1122) -> (element=→"Velcoty_ind_micos":dbl)  [unwired: 1 in]
            n270 = Index Array(array=w1121) -> (element=→"Accele._ind_micos":dbl)  [unwired: 1 in]
            n271 = local read "Signal Segment"() -> (w1136:T3)
            n272 = Bundle By Name(cluster=w1136, "PI_LaserEnergy"=w1131, "Desp_LaserEnergy"=w1130) -> (w1137:T3)
            n273 = call "TriggerRateCalculator.vi"("Count"=w1114) -> ("rep rate"=→"Trig. Rate (Hz)":dbl)  [unwired: 10 in]
            n274 = local write "Signal Segment"(w1137) -> ()
            n275 = global read "Position_ESP300.vi" "Position_ESP"() -> (w1102:dbl[])
            "Position(ESP)" <- w1102
            n276 = global read "Position_ESP300.vi" "Moving"() -> (→"Moving (Newport)":bool)
            n277 = local read "ZeroDelayPos"() -> (w1105:dbl)
            n278 = Index Array(array=w1102) -> (element #1=w1103:dbl, element #2=w1104:dbl)  [unwired: 2 in]
            n279 = Compound Arithmetic op=ADD(w1103, w1104, invert w1105) -> (w1106:dbl)
            n280 = Multiply(x=w1106, y=6.671281903) -> (x*y=→"DP_Delay (ps)_indicator":dbl)
          }
          event "Quit": Value Change; Panel Close; Application Instance Close {
            n281 = event-data() -> ()  [unwired: 1 in, 1 out]
            n282 = Unbundle By Name(w1169) -> ("Apps"=w1170:refnum<queue>)
            n283 = local write "Quit"(FALSE ("Quit")) -> ()
            n284 = Enqueue Element(queue=w1170, element=States-AToF."Quit") -> ()  [unwired: 2 in, 3 out]
            n285 = control-ref of="This VI"() -> (w1166:refnum<vi>)
            n286 = property class="VI"(reference=w1166) -> ("Path"=w1164:path)  [unwired: 1 in, 2 out]
            n287 = Strip Path(path=w1164) -> (stripped path=w1163:path)  [unwired: 1 out]
            n288 = Build Path(base path=w1163, name or relative path=path "Configs/Previous.conf.json" ("ConfigFile Path")) -> (appended path=w1165:path)
            n289 = call "SaveConfigs_toFile.vi"("ConfigFile Path"=w1165, "Configuration"=w1168) -> ()  [unwired: 10 in]
          }
          event Menu Selection (User) {
            n290 = event-data() -> ("ItemTag"=w1178:string, "ItemPath"=w1177:string)  [unwired: 1 in]
            n291 = case shown="\"DepthProfiling(3D)\"" w1178 {
              tunnel: w1177 -> [w1182 _ _ _ _ _ _ _ _ _ _ _ _ _ _ _]
              tunnel: w1176 -> [_ w1186 _ w1210 w1213 w1216 w1218 w1229 w1232 w1235 w1238 w1240 w1245 w1254 _ _]
              tunnel: [_ TRUE _ _ _ _ _ _ _ _ _ _ _ _ _ _] -> w1175
              tunnel: w1174 -> [_ _ w1206 _ _ _ _ _ _ _ _ _ _ _ _ _]
              frame Default {
                n292 = Concatenate Strings(w1182, "\r\n", "This function is not supported by menu yet.") -> (w1181:string)
                n293 = One Button Dialog(message=w1181, button name ("OK")="I know") -> ()  [unwired: 1 out]
              }
              frame "Exit" {
                n294 = Unbundle By Name(w1186) -> ("Apps"=w1185:refnum<queue>)
                n295 = Enqueue Element(queue=w1185, element=States-AToF."Quit") -> ()  [unwired: 2 in, 3 out]
              }
              frame "SaveConfigs" {
                n296 = control-ref of="This VI"() -> (w1199:refnum<vi>)
                n297 = property class="VI"(reference=w1199) -> ("Path"=w1198:path)  [unwired: 1 in, 2 out]
                n298 = Build Path(base path=w1198, name or relative path=".\\Configs\\Default.conf.json") -> (appended path=w1196:path)
                n299 = feedback #2(w1196) -> (w1203:path)
                n300 = Strip Path(path=w1203) -> (stripped path=w1201:path, name=w1202:string)
                n301 = call "File Dialog3"("start path"=w1201, "default name"=w1202, "pattern (all files)"="*.conf.json", "pattern label"="Json Configuration Files") -> ("selected path"=w1189:path, "cancelled"=w1200:bool)  [unwired: 8 in, 2 out]
                n302 = feedback-in #2(w1189) -> ()
                n303 = Strip Path(path=w1189) -> (stripped path=w1191:path, name=w1195:string)
                n304 = Search and Replace String(case sensitive?=TRUE ("ignore case? (F)"), input string=w1195, search string=".conf.json.conf.json", replace string=".conf.json" ("replace string (\"\")")) -> (result string=w1190:string)  [unwired: 4 in, 3 out]
                n305 = Build Path(base path=w1191, name or relative path=w1190) -> (appended path=w1188:path)
                n306 = case shown="False" w1200 {
                  tunnel: w1206 -> [w1208 _]
                  tunnel: w1188 -> [w1207 _]
                  frame False {
                    n307 = call "SaveConfigs_toFile.vi"("ConfigFile Path"=w1207, "Configuration"=w1208) -> ()  [unwired: 10 in]
                  }
                  frame True {
                  }
                }
              }
              frame "EnergyCalibration" {
                n308 = Unbundle By Name(w1210) -> ("Apps"=w1209:refnum<queue>)
                n309 = Enqueue Element(queue=w1209, element=States-AToF."EnergyCalibration") -> ()  [unwired: 2 in, 3 out]
              }
              frame "BeamProfile Measurement" {
                n310 = Unbundle By Name(w1213) -> ("Apps"=w1212:refnum<queue>)
                n311 = Enqueue Element(queue=w1212, element=States-AToF."KnifeEdgeExpt") -> ()  [unwired: 2 in, 3 out]
              }
              frame "DepthProfile" {
                n312 = Unbundle By Name(w1216) -> ("Apps"=w1215:refnum<queue>)
                n313 = Enqueue Element(queue=w1215, element=States-AToF."DepthProfile_RT") -> ()  [unwired: 2 in, 3 out]
              }
              frame "Reset_Micos" {
                n314 = Two Button Dialog(message="Reset Micos? \nHave all subroutines stopped? \nIf not, stop them first. \n", 1:"Cancel" ("F button name (\"Cancel\")"), 2:"Reset Micos" ("T button name (\"OK\")")) -> (T button?=w1222:bool)
                n315 = case shown="True" w1222 {
                  tunnel: w1218 -> [_ w1227]
                  frame False {
                  }
                  frame True {
                    n316 = Unbundle By Name(w1227) -> ("Micos"=w1224:refnum<queue>)
                    n317 = Enqueue Element(queue=w1224, element=T74 {"State"=enum."Close", "Params."=variant}) -> (error out=w1223:errorcluster)  [unwired: 2 in, 2 out]
                    n318 = Enqueue Element(queue=w1224, element=T74 {"State"=enum."Initialize", "Params."=variant}, error in (no error)=w1223) -> ()  [unwired: 1 in, 3 out]
                  }
                }
              }
              frame "Imaging" {
                n319 = Unbundle By Name(w1229) -> ("Apps"=w1228:refnum<queue>)
                n320 = Enqueue Element(queue=w1228, element=States-AToF."Imaging_Micos") -> ()  [unwired: 2 in, 3 out]
              }
              frame "DepthProfiling(3D)" {
                n321 = Unbundle By Name(w1232) -> ("Apps"=w1231:refnum<queue>)
                n322 = Enqueue Element(queue=w1231, element=States-AToF."DepthProfiling(3D)") -> ()  [unwired: 2 in, 3 out]
              }
              frame "BeamProfile Measurement (ESP)" {
                n323 = Unbundle By Name(w1235) -> ("Apps"=w1234:refnum<queue>)
                n324 = Enqueue Element(queue=w1234, element=States-AToF."KnifeEdgeExpt_Npt") -> ()  [unwired: 2 in, 3 out]
              }
              frame "Cleanup Surface" {
                n325 = Unbundle By Name(w1238) -> ("Apps"=w1237:refnum<queue>)
                n326 = Enqueue Element(queue=w1237, element=States-AToF."CleanSurface") -> ()  [unwired: 2 in, 3 out]
              }
              frame "ResetEPM2000" {
                n327 = Unbundle By Name(w1240) -> ("EPM2000"=w1244:refnum<queue>)
                n328 = Enqueue Element(queue=w1244, element=T82 {"State"=enum."Close", "Parameter"=0.0}) -> (queue out=w1243:refnum<queue>)  [unwired: 2 in, 2 out]
                n329 = Enqueue Element(queue=w1243, element=T82 {"State"=enum."Initialize", "Parameter"=0.0}) -> ()  [unwired: 2 in, 3 out]
              }
              frame "ResetBNC" {
                n330 = Unbundle By Name(w1245) -> ("BNC"=w1249:refnum<queue>)
                n331 = Enqueue Element(queue=w1249, element=T83 {"State"=enum."Close", "Para."=variant}) -> (queue out=w1246:refnum<queue>)  [unwired: 2 in, 2 out]
                n332 = Enqueue Element(queue=w1246, element=T83 {"State"=enum."Initialize", "Para."=variant}) -> ()  [unwired: 2 in, 3 out]
              }
              frame "ResetSDGii" {
                n333 = Unbundle By Name(w1254) -> ("SDG_ii"=w1253:refnum<queue>)
                n334 = Enqueue Element(queue=w1253, element=T70 {"State"=enum."Close", "Parameter"=0.0}) -> (queue out=w1250:refnum<queue>)  [unwired: 2 in, 2 out]
                n335 = Enqueue Element(queue=w1250, element=T70 {"State"=enum."Initialize", "Parameter"=0.0}) -> ()  [unwired: 2 in, 3 out]
              }
              frame "SaveCurrentGraph" {
                n336 = control-ref of="Snap"() -> (w1258:refnum<vi>)
                n337 = property class="Bool (strict)"(reference=w1258) -> (reference out=w1255:refnum<vi>, error out=w1256:errorcluster, "Value"=w1257:bool)  [unwired: 1 in]
                n338 = property class="Bool (strict)"(reference=w1255, error in=w1256, "Val(Sgnl)"=w1257) -> ()  [unwired: 2 out]
              }
              frame "MassCalibration", "StartAnalysisTool" {
                n339 = control-ref of="Cali."() -> (w1260:refnum<vi>)
                n340 = vi-ref "AnalysisTools.vi"() -> (w1259:refnum<vi>)
                n341 = call-by-ref "?"(reference=w1259, "Cali.Ref(Caller)"=w1260) -> ()  [unwired: 12 in, 2 out]
              }
            }
          }
          event "Down(ESP)", "Left(ESP)", "Right(ESP)", "Up(ESP)": Value Change {
            n342 = event-data() -> ()  [unwired: 1 in, 1 out]
            n343 = Unbundle By Name(w1280) -> ("ESP300"=w1279:refnum<queue>)
            n344 = Build Array("Up(ESP)", "Down(ESP)", "Left(ESP)", "Right(ESP)") -> (w1274:bool[])
            n345 = Search 1D Array(1D array=w1274, element=TRUE) -> (index of element=w1268:i32)  [unwired: 1 in]
            n346 = Index Array(array=dbl[] [1.0, -1.0, -1.0, 1.0], index=w1268) -> (element=w1271:dbl)
            n347 = Index Array(array=i32[] [2, 2, 1, 1], index=w1268) -> (element=w1272:i32)
            n348 = local read "StepWidth (ESP)"() -> (w1262:T6)
            n349 = Multiply(x=w1271, y=w1262) -> (x*y=w1264:T6)
            n350 = Bundle By Name(cluster=cluster{"Axis":i32, "Position":dbl} {"Axis"=0, "Position"=0.0}, "Position"=w1264, "Axis"=w1272) -> (w1263:cluster{"Axis":i32, "Position":dbl})
            n351 = Bundle By Name(cluster=T74 {"State"=enum."MoveRel", "Params."=variant} ("element"), "Params."=w1263) -> (w1266:T74)
            n352 = Enqueue Element(queue=w1279, element=w1266) -> ()  [unwired: 2 in, 3 out]
          }
          event "Destination(ESP)", "Go(ESP)": Value Change {
            n353 = event-data() -> ()  [unwired: 1 in, 2 out]
            n354 = Unbundle By Name(w1283) -> ("ESP300"=w1282:refnum<queue>)
            n355 = Bundle By Name(cluster=T74 {"State"=enum."MoveAbs_all", "Params."=variant} ("element"), "Params."="Destination(ESP)") -> (w1285:T74)
            n356 = Enqueue Element(queue=w1282, element=w1285) -> ()  [unwired: 2 in, 3 out]
          }
          event "Velocity (ESP)", "Velocity (ESP) #3": Value Change {
            n357 = event-data() -> ()  [unwired: 1 in, 1 out]
            n358 = Unbundle By Name(w1292) -> ("ESP300"=w1291:refnum<queue>)
            n359 = property on="#Axis (ESP300)" class="DigNum (strict)"() -> ("Value"=w1293:i32)  [unwired: 2 in, 2 out]
            n360 = for {
              N: w1293 -> [_]
              tunnel: "Velocity (ESP)" -> [w1299]
              tunnel: w1291 -> [w1301]
              tunnel: "Velocity (ESP) #3" -> [w1300]
              tunnel: [w1295] -> w1287 mode=indexing
              i -> [w1306]
              n361 = Increment(x=w1306) -> (x+1=w1298:i32)
              n362 = Equal?(x=3, y=w1298) -> (x = y?=w1296:bool)
              n363 = Select(t=w1300, s=w1296, f=w1299) -> (s? t:f=w1295:dbl)
              n364 = Bundle By Name(cluster=cluster{"Axis":i32, "Velocity":dbl} {"Axis"=0, "Velocity"=0.0}, "Velocity"=w1295, "Axis"=w1298) -> (w1302:cluster{"Axis":i32, "Velocity":dbl})
              n365 = Bundle By Name(cluster=T74 {"State"=enum."SetVelocity", "Params."=variant} ("element"), "Params."=w1302) -> (w1304:T74)
              n366 = Enqueue Element(queue=w1301, element=w1304) -> ()  [unwired: 2 in, 3 out]
            }
            n367 = Bundle By Name(cluster=w1289, "ESP300.Velocity"=w1287) -> (w1288:T50)
          }
          event "Accele. (ESP)": Value Change {
            n368 = event-data() -> ()  [unwired: 1 in, 2 out]
            n369 = Unbundle By Name(w1311) -> ("ESP300"=w1310:refnum<queue>)
            n370 = property on="#Axis (ESP300)" class="DigNum (strict)"() -> ("Value"=w1313:i32)  [unwired: 2 in, 2 out]
            n371 = for {
              N: w1313 -> [_]
              tunnel: "Accele. (ESP)" -> [w1314]
              tunnel: w1310 -> [w1316]
              tunnel: [w1314] -> w1307 mode=indexing
              i -> [w1321]
              n372 = Increment(x=w1321) -> (x+1=w1320:i32)
              n373 = Bundle By Name(cluster=cluster{"Axis":i32, "Acceleration":dbl} {"Axis"=0, "Acceleration"=0.0}, "Acceleration"=w1314, "Axis"=w1320) -> (w1317:cluster{"Axis":i32, "Acceleration":dbl})
              n374 = Bundle By Name(cluster=T74 {"State"=enum."SetAcceleration", "Params."=variant} ("element"), "Params."=w1317) -> (w1319:T74)
              n375 = Enqueue Element(queue=w1316, element=w1319) -> ()  [unwired: 2 in, 3 out]
            }
            n376 = Bundle By Name(cluster=w1309, "ESP300.Acceleration"=w1307) -> (w1308:T50)
          }
          event "HomeSearch(ESP)": Value Change {
            n377 = event-data() -> ()  [unwired: 1 in, 1 out]
            n378 = Unbundle By Name(w1324) -> ("ESP300"=w1323:refnum<queue>)
            n379 = Enqueue Element(queue=w1323, element=T74 {"State"=enum."Origin/Home", "Params."=variant}) -> ()  [unwired: 2 in, 3 out]
          }
          event "MotorDisabled(ESP)": Value Change {
            n380 = event-data() -> ()  [unwired: 1 in, 1 out]
            n381 = Unbundle By Name(w1331) -> ("ESP300"=w1330:refnum<queue>)
            n382 = Not(x="MotorDisabled(ESP)") -> (.not. x?=w1327:bool)
            n383 = Bundle By Name(cluster=T74 {"State"=enum."MotorEnable(1)", "Params."=variant} ("element"), "Params."=w1327) -> (w1329:T74)
            n384 = Enqueue Element(queue=w1330, element=w1329) -> ()  [unwired: 2 in, 3 out]
          }
          event "STOP(ESP)": Value Change {
            # "think about race condition !!"
            n385 = event-data() -> ()  [unwired: 1 in, 1 out]
            n386 = Unbundle By Name(w1339) -> ("Apps"=w1337:refnum<queue>, "ESP300"=w1338:refnum<queue>)
            n387 = Enqueue Element(queue=w1337, element=States-AToF."Interrupted_Stop") -> (error out=w1335:errorcluster)  [unwired: 2 in, 2 out]
            n388 = call <vilib>:"Clear Errors.vi"("error in (no error)"=w1335) -> ("error out"=w1334:errorcluster)  [unwired: 6 in]
            n389 = Enqueue Element(queue=w1338, element=T74 {"State"=enum."STOP", "Params."=variant}, error in (no error)=w1334) -> ()  [unwired: 1 in, 3 out]
          }
          event User Event {
            n390 = event-data() -> ("Direction"=w1351:i32, "Step"=w1344:i32)  [unwired: 1 in]
            n391 = local read "StepWidth (Micos)"() -> (w1349:T6)
            n392 = Unbundle By Name(w1346) -> ("AppsLock"=w1343:T63, "Micos"=w1354:refnum<queue>, "ESP300"=w1353:refnum<queue>)
            n393 = local read "StepWidth (ESP)"() -> (w1348:T6)
            n394 = Select(t=w1354, s=w1347, f=w1353) -> (s? t:f=w1352:refnum<queue>)
            n395 = Select(t=w1349, s=w1347, f=w1348) -> (s? t:f=w1345:T6)
            n396 = call <vilib>:"Acquire Semaphore.vi"("ms timeout (-1)"=0, "semaphore"=w1343) -> ("timed out"=w1355:bool, "semaphore out"=w1342:T63)  [unwired: 3 in, 1 out]
            n397 = case shown="False" w1355 {
              tunnel: w1352 -> [w1358 _]
              tunnel: w1351 -> [w1362 _]
              tunnel: i32[] [0, 90, 180, 270, -2] -> [w1363 _]
              tunnel: w1345 -> [w1360 _]
              tunnel: w1344 -> [w1359 _]
              tunnel: w1342 -> [w1357 _]
              frame False {
                n398 = Search 1D Array(1D array=w1363, element=w1362) -> (index of element=w1361:i32)  [unwired: 1 in]
                n399 = case shown="0..3" w1361 {
                  selector: w1361 -> [_ w1371]
                  tunnel: w1360 -> [_ w1373]
                  tunnel: w1359 -> [_ w1370]
                  tunnel: w1358 -> [_ w1368]
                  tunnel: w1357 -> [_ w1364]
                  frame Default {
                  }
                  frame 0..3 {
                    n400 = Index Array(array=dbl[] [1.0, -1.0, -1.0, 1.0], index=w1371) -> (element=w1372:dbl)
                    n401 = Index Array(array=i32[] [2, 1, 2, 1], index=w1371) -> (element=w1380:i32)
                    n402 = Compound Arithmetic op=MULTIPLY(w1373, w1372, w1370) -> (w1375:T6)
                    n403 = Bundle By Name(cluster=cluster{"Axis":i32, "Position":dbl} {"Axis"=0, "Position"=0.0}, "Position"=w1375, "Axis"=w1380) -> (w1374:cluster{"Axis":i32, "Position":dbl})
                    n404 = Bundle By Name(cluster=T74 {"State"=enum."MoveRel", "Params."=variant} ("element"), "Params."=w1374) -> (w1369:T74)
                    n405 = Enqueue Element(queue=w1368, element=w1369, timeout in ms (-1)=50) -> (error out=w1365:errorcluster)  [unwired: 1 in, 2 out]
                    n406 = call <vilib>:"Clear Errors.vi"("error in (no error)"=w1365) -> ("error out"=w1366:errorcluster)  [unwired: 6 in]
                    n407 = call <vilib>:"Release Semaphore.vi"("error in (no error)"=w1366, "semaphore"=w1364) -> ()  [unwired: 4 in, 2 out]
                  }
                }
              }
              frame True {
              }
            }
          }
          event User Event {
            w1385 = 1.0  # Pitch
            n408 = event-data() -> ("Direction"=w1391:i32, "Speed"=w1386:dbl)  [unwired: 1 in]
            n409 = Unbundle By Name(w1388) -> ("AppsLock"=w1383:T63, "Micos"=w1394:refnum<queue>, "ESP300"=w1393:refnum<queue>)
            n410 = Select(t=w1394, s=w1389, f=w1393) -> (s? t:f=w1392:refnum<queue>)
            n411 = call <vilib>:"Acquire Semaphore.vi"("ms timeout (-1)"=0, "semaphore"=w1383) -> ("timed out"=w1395:bool, "semaphore out"=w1382:T63)  [unwired: 3 in, 1 out]
            n412 = Select(t=w1385, s=w1389, f=1.0) -> (s? t:f=w1387:dbl)
            n413 = case shown="False" w1395 {
              tunnel: w1392 -> [w1398 _]
              tunnel: w1391 -> [w1399 _]
              tunnel: i32[] [1, 2, 3, 6, -2] -> [w1403 _]
              tunnel: w1387 -> [w1401 _]
              tunnel: w1386 -> [w1400 _]
              tunnel: w1382 -> [w1397 _]
              frame False {
                n414 = Search 1D Array(1D array=w1403, element=w1399) -> (index of element=w1402:i32)  [unwired: 1 in]
                n415 = case shown="0, 1" w1402 {
                  selector: w1402 -> [_ w1413]
                  tunnel: w1401 -> [_ w1415]
                  tunnel: w1400 -> [_ w1416]
                  tunnel: w1399 -> [_ w1414]
                  tunnel: w1398 -> [_ w1408]
                  tunnel: w1397 -> [_ w1405]
                  frame Default {
                  }
                  frame 0, 1 {
                    n416 = Index Array(array=dbl[] [1.0, -1.0], index=w1413) -> (element=w1411:dbl)
                    n417 = Compound Arithmetic op=MULTIPLY(3.0, w1415, w1411, w1416) -> (w1418:dbl)
                    n418 = Bundle By Name(cluster=cluster{"Axis":i32, "Speed(rev/s)":dbl} {"Axis"=0, "Speed(rev/s)"=0.0}, "Speed(rev/s)"=w1418, "Axis"=w1414) -> (w1417:cluster{"Axis":i32, "Speed(rev/s)":dbl})
                    n419 = Bundle By Name(cluster=T74 {"State"=enum."JoyStick", "Params."=variant} ("element"), "Params."=w1417) -> (w1410:T74)
                    n420 = Enqueue Element(queue=w1408, element=w1410, timeout in ms (-1)=0) -> (error out=w1406:errorcluster)  [unwired: 1 in, 2 out]
                    n421 = call <vilib>:"Clear Errors.vi"("error in (no error)"=w1406) -> ("error out"=w1407:errorcluster)  [unwired: 6 in]
                    n422 = call <vilib>:"Release Semaphore.vi"("error in (no error)"=w1407, "semaphore"=w1405) -> ()  [unwired: 4 in, 2 out]
                  }
                }
              }
              frame True {
              }
            }
          }
          event User Event {
            n423 = event-data() -> ()  [unwired: 1 in, 1 out]
            n424 = Unbundle By Name(w1423) -> ("Micos"=w1428:refnum<queue>, "ESP300"=w1427:refnum<queue>)
            n425 = Unbundle By Name(w1423) -> ("AppsLock"=w1424:T63)
            n426 = call <vilib>:"Acquire Semaphore.vi"("ms timeout (-1)"=0, "semaphore"=w1424) -> ("timed out"=w1429:bool, "semaphore out"=w1422:T63)  [unwired: 3 in, 1 out]
            n427 = Select(t=w1428, s=w1425, f=w1427) -> (s? t:f=w1426:refnum<queue>)
            n428 = case shown="False" w1429 {
              tunnel: w1426 -> [w1440 _]
              tunnel: w1422 -> [w1434 _]
              frame False {
                n429 = Enqueue Element(queue=w1440, element=T74 {"State"=enum."STOP", "Params."=variant}) -> (error out=w1435:errorcluster)  [unwired: 2 in, 2 out]
                n430 = call <vilib>:"Clear Errors.vi"("error in (no error)"=w1435) -> ("error out"=w1432:errorcluster)  [unwired: 6 in]
                n431 = call <userlib>:"Wait (ms)__ogtk.vi"("error in (no error)"=w1432, "milliseconds to wait"=u32 250) -> ("error out"=w1433:errorcluster)  [unwired: 8 in, 1 out]
                n432 = call <vilib>:"Release Semaphore.vi"("error in (no error)"=w1433, "semaphore"=w1434) -> ()  [unwired: 4 in, 2 out]
                n433 = feedback #3(0) -> (w1437:i32)
                n434 = Increment(x=w1437) -> (x+1=w1438:i32)
                n435 = feedback-in #3(w1438) -> ()
              }
              frame True {
              }
            }
          }
          event "Up", "Down", "Left", "Right", "Up(+)", "Down(-)", "Left(+)", "Right(-)", "Front", "Back", "Front(-)", "Back(+)": Value Change {
            n436 = event-data() -> ()  [unwired: 1 in, 1 out]
            n437 = Unbundle By Name(w1460) -> ("Micos"=w1459:refnum<queue>, "AppsLock"=w1456:T63)
            n438 = call <vilib>:"Acquire Semaphore.vi"("ms timeout (-1)"=0, "semaphore"=w1456) -> ("timed out"=w1457:bool, "semaphore out"=w1442:T63)  [unwired: 3 in, 1 out]
            n439 = Build Array("Up", "Down", "Left", "Right", "Front", "Back", "Up(+)", "Down(-)", "Left(+)", "Right(-)", "Front(-)", "Back(+)") -> (w1446:bool[])
            n440 = case shown="False" w1457 {
              tunnel: w1459 -> [w1471 _]
              tunnel: w1446 -> [w1464 _]
              tunnel: w1442 -> [w1462 _]
              frame False {
                n441 = Search 1D Array(1D array=w1464, element=TRUE) -> (index of element=w1472:i32)  [unwired: 1 in]
                n442 = local read "StepWidth (Micos)"() -> (w1465:T6)
                n443 = Index Array(array=dbl[] [1.0, -1.0, 1.0, -1.0, -1.0, 1.0, 5.0, -5.0, 5.0, -5.0, -5.0, 5.0], index=w1472) -> (element=w1475:dbl)
                n444 = Index Array(array=i32[] [2, 2, 1, 1, 3, 3, 2, 2, 1, 1, 3, 3], index=w1472) -> (element=w1476:i32)
                n445 = Multiply(x=w1475, y=w1465) -> (x*y=w1467:T6)
                n446 = Bundle By Name(cluster=cluster{"Axis":i32, "Position":dbl} {"Axis"=0, "Position"=0.0}, "Position"=w1467, "Axis"=w1476) -> (w1466:cluster{"Axis":i32, "Position":dbl})
                n447 = Bundle By Name(cluster=T74 {"State"=enum."MoveRel", "Params."=variant} ("element"), "Params."=w1466) -> (w1469:T74)
                n448 = Enqueue Element(queue=w1471, element=w1469) -> (error out=w1461:errorcluster)  [unwired: 2 in, 2 out]
                n449 = call <vilib>:"Clear Errors.vi"("error in (no error)"=w1461) -> ("error out"=w1463:errorcluster)  [unwired: 6 in]
                n450 = call <vilib>:"Release Semaphore.vi"("error in (no error)"=w1463, "semaphore"=w1462) -> ()  [unwired: 4 in, 2 out]
              }
              frame True {
              }
            }
          }
          event "Focus (+)": Value Change {
            n451 = event-data() -> ()  [unwired: 1 in, 1 out]
            n452 = Unbundle By Name(w1484) -> ("Micos"=w1483:refnum<queue>, "AppsLock"=w1480:T63)
            n453 = call <vilib>:"Acquire Semaphore.vi"("ms timeout (-1)"=0, "semaphore"=w1480) -> ("timed out"=w1481:bool, "semaphore out"=w1479:T63)  [unwired: 3 in, 1 out]
            n454 = case shown="False" w1481 {
              tunnel: w1483 -> [w1490 _]
              tunnel: w1479 -> [w1485 _]
              frame False {
                w1488 = 60.0  # Incidence Angle
                n455 = Tangent(1:w1488) -> (0:w1489:dbl)
                n456 = local read "StepWidth (Micos)"() -> (w1496:T6)
                n457 = Build Array(w1489, 0.0 ("element"), 1.0) -> (w1492:dbl[])
                n458 = Multiply(x=w1492, y=w1496) -> (x*y=w1491:T6[])
                n459 = Bundle By Name(cluster=T74 {"State"=enum."MoveRel_all", "Params."=variant} ("element"), "Params."=w1491) -> (w1495:T74)
                n460 = Enqueue Element(queue=w1490, element=w1495) -> (error out=w1486:errorcluster)  [unwired: 2 in, 2 out]
                n461 = call <vilib>:"Clear Errors.vi"("error in (no error)"=w1486) -> ("error out"=w1487:errorcluster)  [unwired: 6 in]
                n462 = call <vilib>:"Release Semaphore.vi"("error in (no error)"=w1487, "semaphore"=w1485) -> ()  [unwired: 4 in, 2 out]
              }
              frame True {
              }
            }
          }
          event "Focus (-)": Value Change {
            n463 = event-data() -> ()  [unwired: 1 in, 1 out]
            n464 = Unbundle By Name(w1500) -> ("Micos"=w1504:refnum<queue>, "AppsLock"=w1501:T63)
            n465 = call <vilib>:"Acquire Semaphore.vi"("ms timeout (-1)"=0, "semaphore"=w1501) -> ("timed out"=w1502:bool, "semaphore out"=w1499:T63)  [unwired: 3 in, 1 out]
            n466 = case shown="False" w1502 {
              tunnel: w1504 -> [w1510 _]
              tunnel: w1499 -> [w1505 _]
              frame False {
                w1508 = -60.0  # Incidence Angle
                n467 = local read "StepWidth (Micos)"() -> (w1516:T6)
                n468 = Tangent(1:w1508) -> (0:w1509:dbl)
                n469 = Build Array(w1509, 0.0 ("element"), -1.0) -> (w1512:dbl[])
                n470 = Multiply(x=w1512, y=w1516) -> (x*y=w1511:T6[])
                n471 = Bundle By Name(cluster=T74 {"State"=enum."MoveRel_all", "Params."=variant} ("element"), "Params."=w1511) -> (w1515:T74)
                n472 = Enqueue Element(queue=w1510, element=w1515) -> (error out=w1506:errorcluster)  [unwired: 2 in, 2 out]
                n473 = call <vilib>:"Clear Errors.vi"("error in (no error)"=w1506) -> ("error out"=w1507:errorcluster)  [unwired: 6 in]
                n474 = call <vilib>:"Release Semaphore.vi"("error in (no error)"=w1507, "semaphore"=w1505) -> ()  [unwired: 4 in, 2 out]
              }
              frame True {
              }
            }
          }
          event "SetFocus": Value Change {
            n475 = event-data() -> ()  [unwired: 1 in, 1 out]
            n476 = Unbundle By Name(w1520) -> ("Micos"=w1519:refnum<queue>)
            n477 = call "SetFocus.vi"() -> ("Aborted?"=w1522:bool, "Destination"=w1521:dbl[])  [unwired: 10 in]
            n478 = case shown="False" w1522 {
              tunnel: w1521 -> [w1524 _]
              tunnel: w1519 -> [w1526 _]
              frame False {
                n479 = property on="Destination" class="Arr (strict)"("Value"=w1524) -> ()  [unwired: 2 in, 2 out]
                n480 = Bundle By Name(cluster=T74 {"State"=enum."MoveAbs_all", "Params."=variant} ("element"), "Params."=w1524) -> (w1523:T74)
                n481 = Enqueue Element(queue=w1526, element=w1523) -> ()  [unwired: 2 in, 3 out]
              }
              frame True {
              }
            }
          }
          event "StopMoving": Value Change {
            n482 = event-data() -> ()  [unwired: 1 in, 1 out]
            n483 = Unbundle By Name(w1534) -> ("Apps"=w1528:refnum<queue>, "Micos"=w1533:refnum<queue>)
            n484 = Enqueue Element(queue=w1528, element=States-AToF."Interrupted_Stop") -> (error out=w1530:errorcluster)  [unwired: 2 in, 2 out]
            n485 = call <vilib>:"Clear Errors.vi"("error in (no error)"=w1530) -> ("error out"=w1529:errorcluster)  [unwired: 6 in]
            n486 = Enqueue Element(queue=w1533, element=T74 {"State"=enum."STOP", "Params."=variant}, error in (no error)=w1529) -> ()  [unwired: 1 in, 3 out]
          }
          event "Home(Micos)": Value Change {
            n487 = event-data() -> ()  [unwired: 1 in, 1 out]
            n488 = Unbundle By Name(w1542) -> ("AppsLock"=w1537:T63, "Micos"=w1538:refnum<queue>)
            n489 = call <vilib>:"Acquire Semaphore.vi"("ms timeout (-1)"=0, "semaphore"=w1537) -> ("timed out"=w1541:bool, "semaphore out"=w1536:T63)  [unwired: 3 in, 1 out]
            n490 = case shown="False" w1541 {
              tunnel: w1538 -> [w1547 _]
              tunnel: T74 {"State"=enum."Origin/Home", "Params."=variant} ("element") -> [w1546 _]
              tunnel: w1536 -> [w1543 _]
              frame False {
                n491 = Enqueue Element(queue=w1547, element=w1546) -> (error out=w1544:errorcluster)  [unwired: 2 in, 2 out]
                n492 = call <vilib>:"Clear Errors.vi"("error in (no error)"=w1544) -> ("error out"=w1545:errorcluster)  [unwired: 6 in]
                n493 = call <vilib>:"Release Semaphore.vi"("error in (no error)"=w1545, "semaphore"=w1543) -> ()  [unwired: 4 in, 2 out]
              }
              frame True {
              }
            }
          }
          event "MoveAbs(Micos)": Value Change {
            n494 = event-data() -> ()  [unwired: 1 in, 1 out]
            n495 = Unbundle By Name(w1558) -> ("AppsLock"=w1555:T63, "Micos"=w1551:refnum<queue>)
            n496 = Bundle By Name(cluster=T74 {"State"=enum."MoveAbs_all", "Params."=variant} ("element"), "Params."="Destination") -> (w1552:T74)
            n497 = property on="MoveAbs(Micos)" class="Bool (strict)"("Value"=FALSE ("MoveAbs(Micos)")) -> ()  [unwired: 2 in, 2 out]
            n498 = call <vilib>:"Acquire Semaphore.vi"("ms timeout (-1)"=0, "semaphore"=w1555) -> ("timed out"=w1556:bool, "semaphore out"=w1550:T63)  [unwired: 3 in, 1 out]
            n499 = case shown="False" w1556 {
              tunnel: w1551 -> [w1563 _]
              tunnel: w1552 -> [w1562 _]
              tunnel: w1550 -> [w1559 _]
              frame False {
                n500 = Enqueue Element(queue=w1563, element=w1562) -> (error out=w1560:errorcluster)  [unwired: 2 in, 2 out]
                n501 = call <vilib>:"Clear Errors.vi"("error in (no error)"=w1560) -> ("error out"=w1561:errorcluster)  [unwired: 6 in]
                n502 = call <vilib>:"Release Semaphore.vi"("error in (no error)"=w1561, "semaphore"=w1559) -> ()  [unwired: 4 in, 2 out]
              }
              frame True {
              }
            }
          }
          event "Position(Micos)": Mouse Down {
            n503 = event-data() -> ("CtlRef"=w1566:refnum<vi>, "Mods.Double Click"=w1567:bool)  [unwired: 1 in]
            n504 = control-ref of="Destination (Micos)"() -> (w1564:refnum<vi>)
            n505 = case shown="True" w1567 {
              tunnel: w1566 -> [_ w1569]
              tunnel: w1564 -> [_ w1568]
              frame False {
              }
              frame True {
                n506 = property on="Property Node" class="Arr (strict)"(reference=w1569) -> ("Value"=w1570:dbl[])  [unwired: 1 in, 2 out]
                n507 = property on="Property Node" class="Arr (strict)"(reference=w1568, "Value"=w1570) -> ()  [unwired: 1 in, 2 out]
              }
            }
          }
          event "Position(ESP)": Mouse Down {
            n508 = event-data() -> ("CtlRef"=w1573:refnum<vi>, "Mods.Double Click"=w1574:bool)  [unwired: 1 in]
            n509 = control-ref of="Destination(ESP)"() -> (w1572:refnum<vi>)
            n510 = case shown="True" w1574 {
              tunnel: w1573 -> [_ w1577]
              tunnel: w1572 -> [_ w1576]
              frame False {
              }
              frame True {
                n511 = property on="Property Node" class="Arr (strict)"(reference=w1577) -> (error out=w1575:errorcluster, "Value"=w1578:dbl[])  [unwired: 1 in, 1 out]
                n512 = property on="Property Node" class="Arr (strict)"(reference=w1576, error in=w1575, "Value"=w1578) -> ()  [unwired: 2 out]
              }
            }
          }
          event "Velocity(Micos)": Value Change {
            n513 = event-data() -> ("NewVal"=w1579:dbl)  [unwired: 1 in]
            n514 = Bundle By Name(cluster=w1581, "Micos.Velocity"=w1579) -> (w1580:T50)
            n515 = Unbundle By Name(w1589) -> ("Micos"=w1584:refnum<queue>)
            n516 = Bundle By Name(cluster=cluster{"Axis":i32, "Velocity":dbl} {"Axis"=1, "Velocity"=0.0}, "Velocity"=w1579) -> (w1585:cluster{"Axis":i32, "Velocity":dbl})
            n517 = Bundle By Name(cluster=T74 {"State"=enum."SetVelocity", "Params."=variant} ("element"), "Params."=w1585) -> (w1587:T74)
            n518 = Enqueue Element(queue=w1584, element=w1587) -> (error out=w1583:errorcluster)  [unwired: 2 in, 2 out]
            n519 = Enqueue Element(queue=w1584, element=T74 {"State"=enum."GetVelocity", "Params."=variant}, error in (no error)=w1583) -> ()  [unwired: 1 in, 3 out]
          }
          event "Accele.(Micos)": Value Change {
            n520 = event-data() -> ("NewVal"=w1590:dbl)  [unwired: 1 in]
            n521 = Bundle By Name(cluster=w1592, "Micos.Acceleration"=w1590) -> (w1591:T50)
            n522 = Bundle By Name(cluster=cluster{"Axis":i32, "Acceleration":dbl} {"Axis"=1, "Acceleration"=0.0}, "Acceleration"=w1590) -> (w1596:cluster{"Axis":i32, "Acceleration":dbl})
            n523 = Unbundle By Name(w1600) -> ("Micos"=w1599:refnum<queue>)
            n524 = Bundle By Name(cluster=T74 {"State"=enum."SetAcceleration", "Params."=variant} ("element"), "Params."=w1596) -> (w1601:T74)
            n525 = Enqueue Element(queue=w1599, element=w1601) -> (queue out=w1595:refnum<queue>, error out=w1594:errorcluster)  [unwired: 2 in, 1 out]
            n526 = Enqueue Element(queue=w1595, element=T74 {"State"=enum."GetAcceleration", "Params."=variant}, error in (no error)=w1594) -> ()  [unwired: 1 in, 3 out]
          }
          event Value Change {
            # "Convert  AnalogDisc's TriggerPosition to Gage's TriggerDelay"
            n527 = event-data() -> ("NewVal"=w1602:T20)  [unwired: 1 in]
            n528 = Unbundle By Name(w1628) -> ("ProcCore_CtrlQueue"=w1621:refnum<queue>, "MainDAQCoreQueue"=w1631:refnum<queue>)
            n529 = Bundle By Name(cluster=w1604, "AnalogDisc_Config"=w1602) -> (w1603:T50)
            n530 = Bundle By Name(cluster=T60 {"DWF States"=enum."SetAll_AcquChTrig_", "Variant"=variant} ("element"), "Variant"=w1602) -> (w1629:T60)
            n531 = Bundle By Name(cluster=T60 {"DWF States"=enum."GetConfig_", "Variant"=variant} ("element"), "Variant"=w1623) -> (w1625:T60)
            n532 = Enqueue Element(queue=w1631, element=w1629) -> (queue out=w1627:refnum<queue>)  [unwired: 2 in, 2 out]
            n533 = Enqueue Element(queue=w1627, element=w1625) -> (error out=w1624:errorcluster)  [unwired: 2 in, 2 out]
            n534 = Dequeue Element(queue=w1623, timeout in ms (-1)=-1, error in (no error)=w1624) -> (element=w1622:T20)  [unwired: 3 out]
            n535 = Unbundle By Name(w1622) -> ("Acqusition.Freq(Hz,SampleRate)"=w1614:dbl, "Acqusition.BufferSize"=w1616:i32, "Trigger.Position(s)"=w1613:dbl)
            n536 = Quotient & Remainder(x=w1616, y=2) -> (floor(x/y)=w1610:i32)  [unwired: 1 out]
            n537 = Reciprocal(x=w1614) -> (1/x=w1612:dbl)
            n538 = Multiply(x=w1612, y=w1610) -> ()  [unwired: 1 out]
            n539 = Divide(x=w1613, y=w1612) -> (x/y=w1609:dbl)
            n540 = Negate(x=w1610) -> (-x=w1611:i32)
            n541 = Subtract(x=w1611, y=w1609) -> (x-y=w1608:dbl)
            n542 = Bundle By Name(cluster=T66 {"TrigDelay"=0.0, "Offset"=0, "Resolution"=-32768, "Range (mV)"=0, "Sample Rate"=100000000.0, "Depth"=16384.0, "Segments"=1} ("DAQParams"), "Sample Rate"=w1614, "Depth"=w1616, "TrigDelay"=w1608) -> (w1618:T66)
            n543 = Bundle By Name(cluster=T75 {"Command"=enum."SetAcquisitionParams", "Params"=variant} ("element"), "Params"=w1618) -> (w1619:T75)
            n544 = Enqueue Element(queue=w1621, element=w1619) -> (queue out=w1607:refnum<queue>)  [unwired: 2 in, 2 out]
            n545 = Enqueue Element(queue=w1607, element=T75 {"Command"=enum."CalcMzArray", "Params"=variant}) -> ()  [unwired: 2 in, 3 out]
          }
          event Value Change {
            n546 = event-data() -> ("NewVal"=w1632:T19, "NewVal.Acquisition.Trigger Delay"=w1646:dbl, "NewVal.Channels"=w1645:T88)  [unwired: 1 in]
            n547 = Unbundle By Name(w1664) -> ("ProcCore_CtrlQueue"=w1659:refnum<queue>, "MainDAQCoreQueue"=w1666:refnum<queue>)
            n548 = Bundle By Name(cluster=T60 {"DWF States"=enum."SetAll_AcquChTrig_", "Variant"=variant} ("element"), "Variant"=w1632) -> (w1637:T60)
            n549 = Build Array(T60 {"DWF States"=enum."GetAll_AcquChTrig", "Variant"=variant} ("element"), T60 {"DWF States"=enum."fStart", "Variant"=variant} ("element"), T60 {"DWF States"=enum."fConfigurate", "Variant"=variant} ("element"), w1637) -> (w1641:T60[])
            n550 = Index Array(array=w1645) -> (element=w1644:T89)  [unwired: 1 in]
            n551 = Reverse 1D Array(array=w1641) -> (reversed array=w1636:T60[])
            n552 = for {
              tunnel: w1636 -> [w1668] mode=indexing
              shift-right: [w1667] -> w1640
              shift-left: w1666 -> [w1669]
              n553 = Enqueue Element(queue=w1669, element=w1668) -> (queue out=w1667:refnum<queue>)  [unwired: 2 in, 2 out]
            }
            n554 = Unbundle By Name(w1644) -> ("Range"=w1643:u32)
            n555 = local read "Signal Segment"() -> (w1648:T3)
            n556 = Bundle By Name(cluster=T60 {"DWF States"=enum."GetConfig_", "Variant"=variant} ("element"), "Variant"=w1649) -> (w1662:T60)
            n557 = Bundle By Name(cluster=w1648, "TrigDelay"=w1646, "DAQ_Range"=w1643) -> (w1647:T3)
            n558 = Enqueue Element(queue=w1640, element=w1662) -> (error out=w1661:errorcluster)  [unwired: 2 in, 2 out]
            n559 = Dequeue Element(queue=w1649, timeout in ms (-1)=-1, error in (no error)=w1661) -> (element=w1660:T19)  [unwired: 3 out]
            n560 = Unbundle By Name(w1660) -> ("Acquisition.Sample Rate"=w1653:dbl, "Acquisition.Depth"=w1654:dbl, "Acquisition.Trigger Delay"=w1650:dbl)
            n561 = local write "Signal Segment"(w1647) -> ()
            n562 = Bundle By Name(cluster=T66 {"TrigDelay"=0.0, "Offset"=0, "Resolution"=-32768, "Range (mV)"=0, "Sample Rate"=100000000.0, "Depth"=16384.0, "Segments"=1} ("DAQParams"), "Sample Rate"=w1653, "Depth"=w1654, "TrigDelay"=w1650) -> (w1656:T66)
            n563 = Bundle By Name(cluster=T75 {"Command"=enum."SetAcquisitionParams", "Params"=variant} ("element"), "Params"=w1656) -> (w1657:T75)
            n564 = Enqueue Element(queue=w1659, element=w1657) -> (queue out=w1652:refnum<queue>)  [unwired: 2 in, 2 out]
            n565 = Bundle By Name(cluster=w1634, "Gage_Config"=w1632) -> (w1633:T50)
            n566 = Enqueue Element(queue=w1652, element=T75 {"Command"=enum."CalcMzArray", "Params"=variant}) -> ()  [unwired: 2 in, 3 out]
          }
          event Value Change {
            # "Removed Configs=>Instrument\nSettings, since GenericDAQ settings need not \nto be saved"
            n567 = event-data() -> ("NewVal"=w1673:T14, "NewVal.Channels"=w1685:cluster{"Range":u32, "DC Offset":i32}[])  [unwired: 1 in]
            n568 = Unbundle By Name(w1701) -> ("ProcCore_CtrlQueue"=w1696:refnum<queue>, "MainDAQCoreQueue"=w1703:refnum<queue>)
            n569 = Bundle By Name(cluster=T60 {"DWF States"=enum."SetAll_AcquChTrig_", "Variant"=variant} ("element"), "Variant"=w1673) -> (w1677:T60)
            n570 = Build Array(T60 {"DWF States"=enum."GetAll_AcquChTrig", "Variant"=variant} ("element"), T60 {"DWF States"=enum."fStart", "Variant"=variant} ("element"), T60 {"DWF States"=enum."fConfigurate", "Variant"=variant} ("element"), w1677) -> (w1681:T60[])
            n571 = Index Array(array=w1685) -> (element=w1684:cluster{"Range":u32, "DC Offset":i32})  [unwired: 1 in]
            n572 = Reverse 1D Array(array=w1681) -> (reversed array=w1676:T60[])
            n573 = for {
              tunnel: w1676 -> [w1705] mode=indexing
              shift-right: [w1704] -> w1680
              shift-left: w1703 -> [w1706]
              n574 = Enqueue Element(queue=w1706, element=w1705) -> (queue out=w1704:refnum<queue>)  [unwired: 2 in, 2 out]
            }
            n575 = Unbundle By Name(w1684) -> ("Range"=w1683:u32)
            n576 = local read "Signal Segment"() -> (w1687:T3)
            n577 = Bundle By Name(cluster=T60 {"DWF States"=enum."GetConfig_", "Variant"=variant} ("element"), "Variant"=w1671) -> (w1699:T60)
            n578 = Bundle By Name(cluster=w1687, "TrigDelay"=0.0, "DAQ_Range"=w1683) -> (w1686:T3)
            n579 = Enqueue Element(queue=w1680, element=w1699) -> (error out=w1698:errorcluster)  [unwired: 2 in, 2 out]
            n580 = Dequeue Element(queue=w1671, timeout in ms (-1)=-1, error in (no error)=w1698) -> (element=w1697:T14)  [unwired: 3 out]
            n581 = Unbundle By Name(w1697) -> ("Acquisition.Sample Rate"=w1690:dbl, "Acquisition.Depth"=w1691:dbl)
            n582 = local write "Signal Segment"(w1686) -> ()
            n583 = Bundle By Name(cluster=T66 {"TrigDelay"=0.0, "Offset"=0, "Resolution"=-32768, "Range (mV)"=0, "Sample Rate"=100000000.0, "Depth"=16384.0, "Segments"=1} ("DAQParams"), "Sample Rate"=w1690, "Depth"=w1691, "TrigDelay"=0.0) -> (w1693:T66)
            n584 = Bundle By Name(cluster=T75 {"Command"=enum."SetAcquisitionParams", "Params"=variant} ("element"), "Params"=w1693) -> (w1694:T75)
            n585 = Enqueue Element(queue=w1696, element=w1694) -> (queue out=w1689:refnum<queue>)  [unwired: 2 in, 2 out]
            n586 = Enqueue Element(queue=w1689, element=T75 {"Command"=enum."CalcMzArray", "Params"=variant}) -> ()  [unwired: 2 in, 3 out]
          }
          event Value Change {
            n587 = event-data() -> ("NewVal"=w1710:T1)  [unwired: 1 in]
            n588 = Unbundle By Name(w1709) -> ("ProcCore_CtrlQueue"=w1708:refnum<queue>)
            n589 = local read "Signal Segment"() -> (w1712:T3)
            n590 = Bundle By Name(cluster=w1712, "Average#"=w1710) -> (w1711:T3)
            n591 = Bundle By Name(cluster=T75 {"Command"=enum."Initialize", "Params"=variant} ("element"), "Command"=ProcessStates."Initialize") -> (w1714:T75)
            n592 = local write "Signal Segment"(w1711) -> ()
            n593 = Enqueue Element(queue=w1708, element=w1714) -> ()  [unwired: 2 in, 3 out]
          }
          event "Rep.Rate (BNC)": Value Change {
            n594 = event-data() -> ("NewVal"=w1716:dbl)  [unwired: 1 in]
            n595 = Unbundle By Name(w1720) -> ("ProcCore_CtrlQueue"=w1719:refnum<queue>)
            n596 = Bundle By Name(cluster=T75 {"Command"=enum."Initialize", "Params"=variant} ("element"), "Params"=w1716, "Command"=ProcessStates."ChangeRepRate") -> (w1722:T75)
            n597 = Enqueue Element(queue=w1719, element=w1722) -> ()  [unwired: 2 in, 3 out]
            n598 = Bundle By Name(cluster=w1718, "Timing(LDPI).RepRate(Hz)"=w1716) -> (w1717:T50)
          }
          event "DisplayIncrement": Value Change {
            n599 = event-data() -> ("NewVal"=w1727:u32)  [unwired: 1 in]
            n600 = Unbundle By Name(w1726) -> ("ProcCore_CtrlQueue"=w1725:refnum<queue>)
            n601 = Bundle By Name(cluster=T75 {"Command"=enum."Initialize", "Params"=variant} ("element"), "Params"=w1727, "Command"=ProcessStates."ChangeDisplayIncrement") -> (w1729:T75)
            n602 = Enqueue Element(queue=w1725, element=w1729) -> ()  [unwired: 2 in, 3 out]
          }
          event "Cali.": Value Change {
            n603 = event-data() -> ("NewVal"=w1731:dbl[])  [unwired: 1 in]
            n604 = Unbundle By Name(w1736) -> ("ProcCore_CtrlQueue"=w1735:refnum<queue>)
            n605 = local read "Signal Segment"() -> (w1738:T3)
            n606 = Bundle By Name(cluster=w1738, "Calibr."=w1731) -> (w1737:T3)
            n607 = local write "Signal Segment"(w1737) -> ()
            n608 = Bundle By Name(cluster=T75 {"Command"=enum."CalcMzArray", "Params"=variant} ("element"), "Params"=w1731) -> (w1734:T75)
            n609 = Enqueue Element(queue=w1735, element=w1734) -> ()  [unwired: 2 in, 3 out]
            n610 = Bundle By Name(cluster=w1733, "Cali."=w1731) -> (w1732:T50)
          }
          event "GraphEnable (A)", "GraphEnable (B)", "IncrementUpdate(A)", "IncrementUpdate(B)", "Resolution(B)", "Resolution(A)": Value Change {
            n611 = event-data() -> ()  [unwired: 1 in, 2 out]
            n612 = Unbundle By Name(w1742) -> ("ProcCore_CtrlQueue"=w1741:refnum<queue>)
            n613 = Enqueue Element At Opposite End(queue=w1741, element=T75 {"Command"=enum."SetGraphsEnable", "Params"=variant}) -> ()  [unwired: 2 in, 3 out]
          }
          event "Binning(A)", "Binning(B)", "BinWidth (A)", "BinWidth (B)": Value Change {
            n614 = event-data() -> ()  [unwired: 1 in, 2 out]
            n615 = Unbundle By Name(w1746) -> ("ProcCore_CtrlQueue"=w1745:refnum<queue>)
            n616 = control-ref of="Binning(B)"() -> (w1755:refnum<vi>)
            n617 = control-ref of="Binning(A)"() -> (w1754:refnum<vi>)
            n618 = property class="Bool (strict)"(reference=w1755) -> ("Value"=w1753:bool)  [unwired: 1 in, 2 out]
            n619 = property class="Bool (strict)"(reference=w1754) -> ("Value"=w1752:bool)  [unwired: 1 in, 2 out]
            n620 = Enqueue Element At Opposite End(queue=w1745, element=T75 {"Command"=enum."SetGraphsEnable", "Params"=variant}) -> ()  [unwired: 2 in, 3 out]
            n621 = control-ref of="Snap"() -> (w1751:refnum<vi>)
            n622 = And(x=w1753, y=w1752) -> (x .and. y?=w1748:bool)
            n623 = Select(t=T49."Disabled and Grayed Out" ("Disabled"), s=w1748, f=T49."Enabled" ("Disabled")) -> (s? t:f=w1747:T49)
            n624 = property class="Bool (strict)"(reference=w1751, "DisabledEnum"=w1747) -> ()  [unwired: 1 in, 2 out]
          }
          event "TopLine", "Baseline", "Threshold", "ZeroOffsetCorrection": Value Change {
            # "Legacy Code, do not follow"
            n625 = event-data() -> ("OldVal"=w1761:variant)  [unwired: 1 in]
            n626 = Unbundle By Name(w1760) -> ("ProcCore_CtrlQueue"=w1759:refnum<queue>)
            n627 = case shown="Default" "Processing Mode" {
              selector: "Processing Mode" -> [w1773 w1783]
              tunnel: w1759 -> [w1781 _]
              tunnel: w1761 -> [_ w1785]
              tunnel: w1758 -> [w1769 w1782]
              tunnel: [w1768 w1782] -> w1757
              frame Default {
                n628 = local read "Processing Mode"() -> (w1763:T4)
                n629 = Build Array("TopLine", "Threshold", "Baseline", "ZeroOffsetCorrection") -> (w1775:dbl[])
                n630 = local read "Threshold"() -> (w1770:dbl)
                n631 = To Variant(anything=w1775) -> (Variant=w1777:variant)
                n632 = Bundle(cluster=cluster{"Processing Mode":T4, "Variant":variant} {"Processing Mode"=enum."None", "Variant"=variant}, "Processing Mode"=w1773, "Variant"=w1777) -> (w1774:cluster{"Processing Mode":T4, "Variant":variant})
                n633 = Bundle By Name(cluster=T75 {"Command"=enum."Initialize", "Params"=variant} ("element"), "Command"=ProcessStates."SetFilterParams", "Params"=w1774) -> (w1779:T75)
                n634 = local read "Signal Segment"() -> (w1772:T3)
                n635 = Enqueue Element(queue=w1781, element=w1779) -> ()  [unwired: 2 in, 3 out]
                n636 = Bundle By Name(cluster=w1772, "ProcMode"=w1763, "Threshold"=w1770) -> (w1771:T3)
                n637 = Bundle By Name(cluster=w1769, "ProcessMethod.TopLine"="TopLine", "ProcessMethod.Threshold"="Threshold", "ProcessMethod.Baseline"="Baseline", "ProcessMethod.ZeroOffset"="ZeroOffsetCorrection", "ProcessMethod.Processing Mode"=w1763) -> (w1768:T50)
                n638 = local write "Signal Segment"(w1771) -> ()
              }
              frame "SetFilter" {
                n639 = Variant To Data(type=w1783, Variant=w1785) -> (data=w1784:T4)  [unwired: 1 in, 1 out]
                n640 = control-ref of="Processing Mode"() -> (w1786:refnum<vi>)
                n641 = property class="Enum (strict)"(reference=w1786, "Value"=w1784) -> ()  [unwired: 1 in, 2 out]
              }
            }
          }
          event "Switch(SDG_II)": Value Change {
            n642 = event-data() -> ()  [unwired: 1 in, 1 out]
            n643 = Unbundle By Name(w1789) -> ("SDG_ii"=w1788:refnum<queue>)
            n644 = Select(t=T70 {"State"=enum."Turn On", "Parameter"=0.0} ("element"), s="Switch(SDG_II)", f=T70 {"State"=enum."Tun OFF", "Parameter"=0.0} ("element")) -> (s? t:f=w1790:T70)
            n645 = Enqueue Element(queue=w1788, element=w1790) -> ()  [unwired: 2 in, 3 out]
          }
          event "Mode(SDG_II)": Value Change {
            n646 = event-data() -> ()  [unwired: 1 in, 1 out]
            n647 = Unbundle By Name(w1797) -> ("SDG_ii"=w1796:refnum<queue>)
            n648 = Select(t=T70 {"State"=enum."Continuous", "Parameter"=0.0} ("element"), s="Mode(SDG_II)", f=T70 {"State"=enum."Single Shot", "Parameter"=0.0} ("element")) -> (s? t:f=w1799:T70)
            n649 = Enqueue Element(queue=w1796, element=w1799) -> ()  [unwired: 2 in, 3 out]
            n650 = Unbundle By Name(w1795) -> ("InstrumentMode.LaserCtrlMethod"=w1794:T17)
            n651 = case shown="\"SDG_II\"" w1794 {
              tunnel: "Mode(SDG_II)" -> [_ w1802]
              frame Default {
              }
              frame "SDG_II" {
                n652 = property on="LaserON" class="Bool (strict)"("Value"=w1802) -> ()  [unwired: 2 in, 2 out]
              }
            }
          }
          event "LaserON": Value Change {
            n653 = event-data() -> ()  [unwired: 1 in, 2 out]
            n654 = Unbundle By Name(w1803) -> ("InstrumentMode.LaserCtrlMethod"=w1805:T17)
            n655 = case shown="\"SRS_DG535\"" w1805 {
              tunnel: "LaserON" -> [w1807 w1808 w1809]
              frame "SDG_II" {
                n656 = property on="Mode(SDG_II)" class="Bool (strict)"("Val(Sgnl)"=w1807) -> ()  [unwired: 2 in, 2 out]
              }
              frame "BNC" {
                n657 = property on="BNC On/Off" class="Bool (strict)"("Val(Sgnl)"=w1808) -> ()  [unwired: 2 in, 2 out]
              }
              frame "SRS_DG535" {
                n658 = property on="SRS On/Off" class="Bool (strict)"("Val(Sgnl)"=w1809) -> ()  [unwired: 2 in, 2 out]
              }
            }
            n659 = disable-structure shown="Disabled" {
              disable-tunnel: "LaserON" -> [w1806 _]
              frame Disabled {
                # "^For Emulation only"
                n660 = global write "Emu_CoreDAQ_Globle.vi" "Enable"(w1806) -> ()
              }
              frame Enabled {
              }
            }
          }
          event "ManlTrig(SDG)": Value Change {
            n661 = event-data() -> ()  [unwired: 1 in, 1 out]
            n662 = Unbundle By Name(w1812) -> ("SDG_ii"=w1811:refnum<queue>)
            n663 = Enqueue Element(queue=w1811, element=T70 {"State"=enum."ManualTrigger", "Parameter"=0.0}) -> ()  [unwired: 2 in, 3 out]
          }
          event "Meander", "DepthProfile", "Set dbl pulse Delay", "Meander (ESP)", "DelayScan", "BeamProfiling(ESP)": Value Change {
            w1826 = T71[] [enum."Meander_MCS", enum."DepthProfiling", enum."DelayScan", enum."Set_2PulseDelay", enum."Meander_Npt", enum."KnifeEdgeExpt_Npt"] items=["Initialize", "Idle", "CalcMzArray", "Meander_SGL_MCS", "Meander_MCS", "CleanSurface", "Meander_Npt", "Meander_SGL_Npt", "KnifeEdgeExpt", "KnifeEdgeExpt_Npt", "Imaging_Micos", "Imaging_ESP", "DepthProfiling", "Set_2PulseDelay", "DelayScan", "PeakSearch", "ExportOrigin", "Save Settings", "Load Settings", "Save as Default", "Load Default", "EnergyCalibration", "Quit", "Interrupted_Stop", "Quit_SubProgram", "StepMove_Joystick", "ContMove_Joystick", "Stop_Joystick", "Check_AppsLock", "Return_Status", "DepthProfile_RT", "UpdateInstruStates", "InstruOptimizer_static", "InstruOptimizer_dynamic", "DepthProfiling(3D)"]
            n664 = event-data() -> ()  [unwired: 1 in, 1 out]
            n665 = Unbundle By Name(w1828) -> ("Apps"=w1827:refnum<queue>)
            n666 = Build Array("Meander", "DepthProfile", "DelayScan", "Set dbl pulse Delay", "Meander (ESP)", "BeamProfiling(ESP)") -> (w1823:bool[])
            n667 = global read "Position_Micos.vi" "Moving(Micos)"() -> (w1816:bool)
            n668 = global read "Position_ESP300.vi" "Moving"() -> (w1814:bool)
            n669 = Or(x=w1816, y=w1814) -> (x .or. y?=w1815:bool)
            n670 = Build Array(w1816, w1816, w1815, w1814, w1814, w1816) -> (w1817:bool[])
            n671 = for {
              tunnel: w1827 -> [w1833]
              tunnel: w1826 -> [w1831] mode=indexing
              tunnel: w1823 -> [w1830] mode=indexing
              tunnel: w1817 -> [w1829] mode=indexing
              n672 = Compound Arithmetic op=AND(invert w1829, w1830) -> (w1832:bool)
              n673 = case shown="True" w1832 {
                tunnel: w1833 -> [_ w1835]
                tunnel: w1831 -> [_ w1834]
                frame False {
                }
                frame True {
                  n674 = Enqueue Element(queue=w1835, element=w1834) -> ()  [unwired: 2 in, 3 out]
                }
              }
            }
          }
          event "Pause": Value Change {
            n675 = event-data() -> ()  [unwired: 1 in, 1 out]
            n676 = global write "PauseMeander.vi" "Pause Meaner"("Pause") -> ()
            n677 = property on="Pause" class="Bool (strict)"("Blinking"="Pause") -> ()  [unwired: 2 in, 2 out]
          }
          event "BNC On/Off": Value Change {
            n678 = event-data() -> ()  [unwired: 1 in, 2 out]
            n679 = Unbundle By Name(w1845) -> ("BNC"=w1844:refnum<queue>)
            n680 = Select(t=T83 {"State"=enum."Run", "Para."=variant} ("element"), s="BNC On/Off", f=T83 {"State"=enum."Stop", "Para."=variant} ("element")) -> (s? t:f=w1841:T83)
            n681 = Enqueue Element(queue=w1844, element=w1841) -> ()  [unwired: 2 in, 3 out]
            n682 = Unbundle By Name(w1839) -> ("InstrumentMode.LaserCtrlMethod"=w1840:T17)
            n683 = case shown="\"BNC\"" w1840 {
              tunnel: "BNC On/Off" -> [_ w1846]
              frame Default {
              }
              frame "BNC" {
                n684 = property on="LaserON" class="Bool (strict)"("Value"=w1846) -> ()  [unwired: 2 in, 2 out]
              }
            }
          }
          event "Set Mode": Value Change {
            n685 = event-data() -> ()  [unwired: 1 in, 1 out]
            n686 = Unbundle By Name(w1868) -> ("BNC"=w1867:refnum<queue>)
            n687 = Unbundle By Name(w1864) -> ("InstrumentMode.LaserCtrlMethod"=w1866:T17)
            n688 = property on="BNC On/Off" class="Bool (strict)"("Value"=FALSE ("BNC Switch")) -> ()  [unwired: 2 in, 2 out]
            n689 = case shown="\"BNC\"" w1866 {
              tunnel: FALSE -> [_ w1884]
              frame Default {
              }
              frame "BNC" {
                n690 = property on="LaserON" class="Bool (strict)"("Value"=w1884) -> ()  [unwired: 2 in, 2 out]
              }
            }
            n691 = Bundle By Name(cluster=T86 {"Rep.Rate"=0.0, "Sys Ext Mode"=enum."Triggered", "Mode"=enum."Normal"}, "Mode"="Mode (BNC)", "Rep.Rate"="Rep.Rate (BNC)", "Sys Ext Mode"="Trigger Mode (BNC)") -> (w1860:T86)
            n692 = Bundle By Name(cluster=w1864, "BNC_Config.System.Mode"="Mode (BNC)", "BNC_Config.System.Rep.Rate"="Rep.Rate (BNC)", "BNC_Config.System.Sys Ext Mode"="Trigger Mode (BNC)") -> (w1851:T50)
            n693 = To Variant(anything=w1860) -> (Variant=w1861:variant)
            n694 = Bundle By Name(cluster=T83 {"State"=enum."Set System", "Para."=variant} ("element"), "Para."=w1861) -> (w1859:T83)
            n695 = Enqueue Element(queue=w1867, element=w1859) -> (error out=w1862:errorcluster)  [unwired: 2 in, 2 out]
            n696 = Unbundle By Name(w1851) -> ("BNC_Config.Channels"=w1850:T33[])
            n697 = for {
              N -> [w1871]
              tunnel: w1867 -> [w1883]
              tunnel: "Channels Enable Status" -> [w1873] mode=indexing
              shift-right: [w1876] -> _
              shift-left: w1862 -> [w1882]
              tunnel: w1850 -> [w1874] mode=indexing
              tunnel: [w1872] -> w1849 mode=indexing
              tunnel: [w1871] -> w1847
              i -> [w1877]
              n698 = Increment(x=w1877) -> (x+1=w1875:i32)
              n699 = Bundle By Name(cluster=T37 {"Channel"=0, "Enable"=FALSE}, "Channel"=w1875, "Enable"=w1873) -> (w1879:T37)
              n700 = Bundle By Name(cluster=w1874, "C-Enables.Enable"=w1873) -> (w1872:T33)
              n701 = Bundle By Name(cluster=T83 {"State"=enum."Set C-Enable", "Para."=variant} ("element"), "Para."=w1879) -> (w1880:T83)
              n702 = Enqueue Element(queue=w1883, element=w1880, error in (no error)=w1882) -> (error out=w1876:errorcluster)  [unwired: 1 in, 2 out]
            }
            n703 = in-place {
              in-place-border: w1849 -> [w1869]
              n704 = in-place-split #4(w1850, w1847) -> (w1870:T33[])  [unwired: 1 out]
              n705 = in-place-split #4(w1869, w1870) -> (w1848:T33[])  [unwired: 1 out]
            }
            n706 = Bundle By Name(cluster=w1851, "BNC_Config.Channels"=w1848) -> (w1863:T50)
          }
          event "Delay B", "Width A", "Width B", "Delay A": Value Change {
            # "legacy, need improvement"
            n707 = event-data() -> ()  [unwired: 1 in, 2 out]
            n708 = Unbundle By Name(w1894) -> ("BNC"=w1893:refnum<queue>)
            n709 = Unbundle By Name(w1889) -> ("BNC_Config.Channels"=w1888:T33[])
            n710 = Build Array("Delay A", "Delay B") -> (w1892:dbl[])
            n711 = Build Array("Width A", "Width B") -> (w1891:dbl[])
            n712 = for {
              N -> [w1901]
              tunnel: w1893 -> [w1912]
              tunnel: w1892 -> [w1907] mode=indexing
              tunnel: w1891 -> [w1906] mode=indexing
              tunnel: w1888 -> [w1904] mode=indexing
              tunnel: [w1902] -> w1885 mode=indexing
              tunnel: [w1901] -> w1886
              i -> [w1908]
              w1903 = T35 {"Channel"=0, "Delay"=0.0, "Width"=0.0}  # Set C-Mode
              n713 = Increment(x=w1908) -> (x+1=w1905:i32)
              n714 = Bundle By Name(cluster=w1903, "Channel"=w1905, "Delay"=w1907, "Width"=w1906) -> (w1909:T35)
              n715 = Bundle By Name(cluster=T83 {"State"=enum."Set C-Mode", "Para."=variant} ("element"), "Para."=w1909) -> (w1910:T83)
              n716 = Bundle By Name(cluster=w1904, "C-Mode"=w1903) -> (w1902:T33)
              n717 = Enqueue Element(queue=w1912, element=w1910) -> ()  [unwired: 2 in, 3 out]
            }
            n718 = in-place {
              in-place-border: w1885 -> [w1899]
              n719 = in-place-split #5(w1888, w1886) -> (w1900:T33[])  [unwired: 1 out]
              n720 = in-place-split #5(w1899, w1900) -> (w1887:T33[])  [unwired: 1 out]
            }
            n721 = Bundle By Name(cluster=w1889, "BNC_Config.Channels"=w1887) -> (w1890:T50)
          }
          event "Ch_A", "Ch_B", "Ch_C", "Ch_D": Value Change {
            n722 = event-data() -> ()  [unwired: 1 in, 2 out]
            n723 = Unbundle By Name(w1924) -> ("SRS DG535"=w1923:refnum<queue>)
            n724 = property on="DG535_Configs" class="Clust (strict)"() -> ("Value"=w1916:T48)  [unwired: 2 in, 2 out]
            n725 = Build Array("Ch_A", "Ch_B", "Ch_C", "Ch_D") -> (w1918:dbl[])
            n726 = Unbundle By Name(w1916) -> ("Delays"=w1917:T28[])
            n727 = for {
              tunnel: w1923 -> [w1931]
              tunnel: w1918 -> [w1927] mode=indexing
              shift-right: [w1929] -> _
              shift-left: _ -> [w1928]
              tunnel: w1917 -> [w1926] mode=indexing
              tunnel: [w1925] -> w1913 mode=indexing
              n728 = call-poly <userlib>:"Data Changed__ogtk.vi"("DBL"=w1927) -> ("Changed"=w1930:bool)
              n729 = case shown="True" w1930 {
                tunnel: w1931 -> [_ w1944]
                tunnel: [w1933 w1941] -> w1929
                tunnel: w1928 -> [w1933 w1940]
                tunnel: w1927 -> [_ w1939]
                tunnel: w1926 -> [w1932 w1937]
                tunnel: [w1932 w1934] -> w1925
                frame False {
                }
                frame True {
                  n730 = Unbundle By Name(w1937) -> ("Channel"=w1936:T29, "Sync To"=w1935:T29)
                  n731 = Bundle By Name(cluster=T28 {"Channel"=enum."A Output", "Sync To"=enum."T0 Output", "Delay"=0.0}, "Channel"=w1936, "Sync To"=w1935, "Delay"=w1939) -> (w1934:T28)
                  n732 = Bundle By Name(cluster=T81 {"State"=enum."Set Delay", "Para."=variant} ("element"), "Para."=w1934) -> (w1942:T81)
                  n733 = Enqueue Element(queue=w1944, element=w1942, error in (no error)=w1940) -> (error out=w1941:errorcluster)  [unwired: 1 in, 2 out]
                }
              }
            }
            n734 = Bundle By Name(cluster=w1915, "DG535.Delays"=w1913) -> (w1914:T50)
          }
          event "Delay(LDI-Rej.)", "Delay(PI)": Value Change {
            n735 = event-data() -> ()  [unwired: 1 in, 1 out]
            n736 = Unbundle By Name(w1950) -> ("Timing(LDPI).NoDelayOffset"=w1949:dbl, "InstrumentMode.InstruMode"=w1948:T18)
            n737 = Bundle By Name(cluster=w1950, "Timing(LDPI).Delay(PI)"="Delay(PI)", "Timing(LDPI).Delay(Rejection)"="Delay(LDI-Rej.)") -> (w1947:T50)
            n738 = case shown="\"fsLDPI\"" w1948 {
              tunnel: "Delay(PI)" -> [w1957 w1964 w1971 _ _ _]
              tunnel: "Delay(LDI-Rej.)" -> [w1956 w1963 w1970 _ _ _]
              tunnel: w1949 -> [w1951 w1962 w1969 _ _ _]
              frame "fsLDPI" {
                # "NoDelayOffset: 99.8095m"
                # "Ch_A=> 0 delay offset\nCh_B => ND:YAG flashlamp\n-CD HV pulser\n\nND:YAG Sync => Gage Trig in"
                n739 = First Call?() -> (First Call?: T/F=w1952:bool)
                n740 = Add(x=w1957, y=w1956) -> (x+y=w1954:dbl)
                n741 = case shown="True" w1952 {
                  tunnel: w1951 -> [_ w1958]
                  frame False {
                  }
                  frame True {
                    n742 = control-ref of="Ch_A"() -> (w1960:refnum<vi>)
                    n743 = control-ref of="Ch_C"() -> (w1959:refnum<vi>)
                    n744 = property class="DigNum (strict)"(reference=w1960, "Val(Sgnl)"=w1958) -> ()  [unwired: 1 in, 2 out]
                    n745 = property class="DigNum (strict)"(reference=w1959, "Val(Sgnl)"=0.0 ("Value (Signaling)")) -> ()  [unwired: 1 in, 2 out]
                  }
                }
                n746 = control-ref of="Ch_B"() -> (w1953:refnum<vi>)
                n747 = control-ref of="Ch_D"() -> (w1955:refnum<vi>)
                n748 = property class="DigNum (strict)"(reference=w1955, "Val(Sgnl)"=w1954) -> ()  [unwired: 1 in, 2 out]
                n749 = property class="DigNum (strict)"(reference=w1953, "Val(Sgnl)"=w1957) -> ()  [unwired: 1 in, 2 out]
              }
              frame "nsLDPI" {
                # "NoDelayOffset: 0.0001766"
                # "T0 => ND:YAG flashlap, inverted, High-Z\nCh_A => Explorer trig in, inverted\nCh_B => \nCh_D => HV pulser rise\n-CD => HV pulse"
                n750 = Add(x=w1964, y=w1963) -> (x+y=w1967:dbl)
                n751 = Subtract(x=w1962, y=w1964) -> (x-y=w1966:dbl)
                n752 = control-ref of="Ch_A"() -> (w1965:refnum<vi>)
                n753 = control-ref of="Ch_D"() -> (w1968:refnum<vi>)
                n754 = property class="DigNum (strict)"(reference=w1968, "Val(Sgnl)"=w1967) -> ()  [unwired: 1 in, 2 out]
                n755 = property class="DigNum (strict)"(reference=w1965, "Val(Sgnl)"=w1966) -> ()  [unwired: 1 in, 2 out]
              }
              frame "nsLD-fsPI" {
                (unwired) 0.0009859
                n756 = Negate(x=w1971) -> (-x=w1972:dbl)
                n757 = Add(x=0.001, y=w1970) -> (x+y=w1978:dbl)
                n758 = control-ref of="Ch_A"() -> (w1975:refnum<vi>)
                n759 = control-ref of="Ch_B"() -> (w1977:refnum<vi>)
                n760 = control-ref of="Ch_D"() -> (w1979:refnum<vi>)
                n761 = control-ref of="Ch_C"() -> (w1976:refnum<vi>)
                n762 = property class="DigNum (strict)"(reference=w1979, "Val(Sgnl)"=w1978) -> ()  [unwired: 1 in, 2 out]
                n763 = property class="DigNum (strict)"(reference=w1976, "Val(Sgnl)"=5e-05 ("Value (Signaling)")) -> ()  [unwired: 1 in, 2 out]
                n764 = property class="DigNum (strict)"(reference=w1975, "Val(Sgnl)"=w1969) -> ()  [unwired: 1 in, 2 out]
                n765 = property class="DigNum (strict)"(reference=w1977, "Val(Sgnl)"=w1972) -> ()  [unwired: 1 in, 2 out]
              }
              frame "GenericTOF" {
                n766 = First Call?() -> (First Call?: T/F=w1980:bool)
                n767 = case shown="True" w1980 {
                  frame False {
                  }
                  frame True {
                    w1981 = 0.0 ("Value (Signaling)")
                    n768 = control-ref of="Ch_B"() -> (w1982:refnum<vi>)
                    n769 = control-ref of="Ch_D"() -> (w1983:refnum<vi>)
                    n770 = control-ref of="Ch_A"() -> (w1985:refnum<vi>)
                    n771 = control-ref of="Ch_C"() -> (w1984:refnum<vi>)
                    n772 = property class="DigNum (strict)"(reference=w1982, "Val(Sgnl)"=w1981) -> ()  [unwired: 1 in, 2 out]
                    n773 = property class="DigNum (strict)"(reference=w1983, "Val(Sgnl)"=w1981) -> ()  [unwired: 1 in, 2 out]
                    n774 = property class="DigNum (strict)"(reference=w1985, "Val(Sgnl)"=w1981) -> ()  [unwired: 1 in, 2 out]
                    n775 = property class="DigNum (strict)"(reference=w1984, "Val(Sgnl)"=w1981) -> ()  [unwired: 1 in, 2 out]
                  }
                }
              }
              frame "BeamProfiling" {
                n776 = First Call?() -> (First Call?: T/F=w1986:bool)
                n777 = case shown="True" w1986 {
                  frame False {
                  }
                  frame True {
                    w1987 = 0.0 ("Value (Signaling)")
                    n778 = control-ref of="Ch_B"() -> (w1988:refnum<vi>)
                    n779 = control-ref of="Ch_D"() -> (w1989:refnum<vi>)
                    n780 = control-ref of="Ch_A"() -> (w1991:refnum<vi>)
                    n781 = control-ref of="Ch_C"() -> (w1990:refnum<vi>)
                    n782 = property class="DigNum (strict)"(reference=w1988, "Val(Sgnl)"=w1987) -> ()  [unwired: 1 in, 2 out]
                    n783 = property class="DigNum (strict)"(reference=w1989, "Val(Sgnl)"=w1987) -> ()  [unwired: 1 in, 2 out]
                    n784 = property class="DigNum (strict)"(reference=w1991, "Val(Sgnl)"=w1987) -> ()  [unwired: 1 in, 2 out]
                    n785 = property class="DigNum (strict)"(reference=w1990, "Val(Sgnl)"=w1987) -> ()  [unwired: 1 in, 2 out]
                  }
                }
              }
              frame Default {
                n786 = First Call?() -> (First Call?: T/F=w1992:bool)
                n787 = case shown="True" w1992 {
                  frame False {
                  }
                  frame True {
                    w1993 = 0.0 ("Value (Signaling)")
                    n788 = control-ref of="Ch_B"() -> (w1994:refnum<vi>)
                    n789 = control-ref of="Ch_D"() -> (w1995:refnum<vi>)
                    n790 = control-ref of="Ch_A"() -> (w1997:refnum<vi>)
                    n791 = control-ref of="Ch_C"() -> (w1996:refnum<vi>)
                    n792 = property class="DigNum (strict)"(reference=w1994, "Val(Sgnl)"=w1993) -> ()  [unwired: 1 in, 2 out]
                    n793 = property class="DigNum (strict)"(reference=w1995, "Val(Sgnl)"=w1993) -> ()  [unwired: 1 in, 2 out]
                    n794 = property class="DigNum (strict)"(reference=w1997, "Val(Sgnl)"=w1993) -> ()  [unwired: 1 in, 2 out]
                    n795 = property class="DigNum (strict)"(reference=w1996, "Val(Sgnl)"=w1993) -> ()  [unwired: 1 in, 2 out]
                  }
                }
              }
            }
          }
          event "Internal/Burst Rate": Value Change {
            n796 = event-data() -> ()  [unwired: 1 in, 2 out]
            n797 = Unbundle By Name(w2008) -> ("SRS DG535"=w2007:refnum<queue>)
            n798 = property on="DG535_Configs" class="Clust (strict)"() -> ("Value"=w2003:T48)  [unwired: 2 in, 2 out]
            n799 = Unbundle By Name(w2003) -> ("Trigger"=w2002:T27)
            n800 = Bundle By Name(cluster=w2002, "Internal/Burst Rate"="Internal/Burst Rate", "Trigger Mode"="Trigger Mode (SRS)") -> (w1999:T27)
            n801 = Bundle By Name(cluster=T81 {"State"=enum."Set Trigger", "Para."=variant} ("element"), "Para."=w1999) -> (w2005:T81)
            n802 = Bundle By Name(cluster=w2001, "Timing(LDPI).RepRate(Hz)"="Internal/Burst Rate", "DG535.Trigger"=w1999) -> (w2000:T50)
            n803 = Enqueue Element(queue=w2007, element=w2005) -> ()  [unwired: 2 in, 3 out]
          }
          event "SRS On/Off": Value Change {
            n804 = event-data() -> ()  [unwired: 1 in, 2 out]
            n805 = Unbundle By Name(w2019) -> ("SRS DG535"=w2018:refnum<queue>)
            n806 = Select(t=T81 {"State"=enum."Run", "Para."=variant} ("element"), s="SRS On/Off", f=T81 {"State"=enum."Stop", "Para."=variant}) -> (s? t:f=w2017:T81)
            n807 = Enqueue Element(queue=w2018, element=w2017) -> ()  [unwired: 2 in, 3 out]
            n808 = Unbundle By Name(w2012) -> ("DG535.Trigger.Trigger Mode"=w2010:T7, "InstrumentMode.LaserCtrlMethod"=w2014:T17)
            n809 = Equal?(x=DG535_TriggerMode."Internal" ("DG535.Trigger.Trigger Mode"), y=w2010) -> (x = y?=w2009:bool)
            n810 = case shown="True" w2009 {
              tunnel: w2014 -> [_ w2021]
              tunnel: "SRS On/Off" -> [_ w2020]
              frame False {
              }
              frame True {
                n811 = case shown="\"BNC\"" w2021 {
                  tunnel: w2020 -> [_ w2022]
                  frame Default {
                  }
                  frame "BNC" {
                    n812 = property on="LaserON" class="Bool (strict)"("Value"=w2022) -> ()  [unwired: 2 in, 2 out]
                  }
                }
              }
            }
          }
          event "Record": Value Change {
            n813 = event-data() -> ("NewVal"=w2027:bool)  [unwired: 1 in]
            n814 = Unbundle By Name(w2026) -> ("ProcCore_CtrlQueue"=w2025:refnum<queue>, "WriterCtrl"=w2024:refnum<queue>)
            n815 = case shown="True" w2027 {
              tunnel: w2024 -> [w2035 w2048]
              tunnel: w2025 -> [w2029 w2040]
              frame False {
                n816 = Bundle By Name(cluster=T75 {"Command"=enum."Initialize", "Params"=variant} ("element"), "Command"=ProcessStates."StopSave") -> (w2031:T75)
                n817 = Enqueue Element(queue=w2029, element=w2031) -> (error out=w2028:errorcluster)  [unwired: 2 in, 2 out]
                n818 = Enqueue Element(queue=w2035, element=T68 {"State"=enum."Close", "Params"=variant}, error in (no error)=w2028) -> ()  [unwired: 1 in, 3 out]
                n819 = property on="Snap" class="Bool (strict)"("DisabledEnum"=T49."Enabled" ("Disabled")) -> ()  [unwired: 2 in, 2 out]
              }
              frame True {
                n820 = local read "Files Format"() -> (w2038:T2)
                n821 = call <vilib>:"Dflt Data Dir.vi"() -> ("App:Default Data Directory"=w2036:path)
                n822 = Index Array(array=string[] ["*.txt", "*.mzml", "*.bin", "*.img", "*.imzML"], index=w2038) -> (element=w2037:string)
                n823 = feedback #6(w2036) -> (w2041:path)
                n824 = Strip Path(path=w2041) -> (stripped path=w2044:path, name=w2043:string)
                n825 = call "File Dialog2"("start path"=w2044, "default name"=w2043, "pattern (all files)"=w2037) -> ("selected path"=w2045:path, "cancelled"=w2047:bool, "error out"=w2046:errorcluster)  [unwired: 9 in, 1 out]
                n826 = case shown="False" w2047 {
                  tunnel: w2048 -> [w2057 _]
                  tunnel: w2045 -> [w2053 _]
                  tunnel: w2046 -> [_ _]
                  tunnel: [w2053 w2059] -> w2042
                  tunnel: w2041 -> [_ w2059]
                  tunnel: w2040 -> [w2052 _]
                  frame False {
                    n827 = local write "Filename Indicator"(w2053) -> ()
                    n828 = Bundle By Name(cluster=T75 {"Command"=enum."Initialize", "Params"=variant} ("element"), "Command"=ProcessStates."StartSave") -> (w2050:T75)
                    n829 = Bundle By Name(cluster=T68 {"State"=enum."Open", "Params"=variant} ("element"), "Params"=w2053) -> (w2055:T68)
                    n830 = property on="Snap" class="Bool (strict)"("DisabledEnum"=T49."Disabled and Grayed Out" ("Disabled")) -> ()  [unwired: 2 in, 2 out]
                    n831 = Enqueue Element(queue=w2052, element=w2050) -> ()  [unwired: 2 in, 3 out]
                    n832 = Enqueue Element(queue=w2057, element=w2055) -> ()  [unwired: 2 in, 3 out]
                  }
                  frame True {
                    n833 = property on="Record" class="Bool (strict)"("Value"=FALSE ("Save Multiple")) -> ()  [unwired: 2 in, 2 out]
                  }
                }
                n834 = feedback-in #6(w2042) -> ()
              }
            }
          }
          event "Snap": Value Change {
            n835 = event-data() -> ()  [unwired: 1 in, 1 out]
            n836 = local read "IncrementUpdate(A)"() -> (w2067:bool)
            n837 = local read "IncrementUpdate(B)"() -> (w2071:bool)
            n838 = local read "GraphEnable (A)"() -> (w2069:bool)
            n839 = local read "GraphEnable (B)"() -> (w2072:bool)
            n840 = Unbundle By Name(w2063) -> ("WriterCtrl"=w2062:refnum<queue>, "WriterSIG"=w2061:refnum<queue>)
            n841 = local read "Binning(A)"() -> (w2068:bool)
            n842 = local read "Binning(B)"() -> (w2070:bool)
            n843 = Compound Arithmetic op=AND(w2072, invert w2070, invert w2071) -> (w2064:bool)
            n844 = Compound Arithmetic op=AND(w2069, invert w2068, invert w2067) -> (w2065:bool)
            n845 = Or(x=w2064, y=w2065) -> (x .or. y?=w2066:bool)
            n846 = case shown="True" w2066 {
              tunnel: w2064 -> [_ w2092]
              tunnel: w2062 -> [_ w2090]
              tunnel: w2061 -> [_ w2089]
              tunnel: [_ w2085] -> w2073
              frame False {
                n847 = One Button Dialog(message="No active graph windows, no file is saved.\nPlease active one graph before press \"Save Once\"") -> ()  [unwired: 1 in, 1 out]
              }
              frame True {
                n848 = call <vilib>:"Dflt Data Dir.vi"() -> ("App:Default Data Directory"=w2076:path)
                n849 = local read "Graph (B)"() -> (w2086:cluster{dbl[], dbl[]})
                n850 = local read "Graph (A)"() -> (w2087:cluster{dbl[], dbl[]})
                n851 = Select(t=w2086, s=w2092, f=w2087) -> (s? t:f=w2088:cluster{dbl[], dbl[]})
                n852 = feedback #7(w2076) -> (w2078:path)
                n853 = Strip Path(path=w2078) -> (stripped path=w2082:path, name=w2081:string)
                n854 = call "File Dialog"("start path"=w2082, "default name"=w2081, "pattern (all files)"="*.txt", "pattern label"="Text MS File") -> ("selected path"=w2080:path, "cancelled"=w2091:bool, "error out"=w2077:errorcluster)  [unwired: 8 in, 1 out]
                n855 = case shown="False" w2091 {
                  tunnel: w2090 -> [_ _]
                  tunnel: w2080 -> [w2096 _]
                  tunnel: w2089 -> [_ _]
                  tunnel: w2088 -> [w2101 _]
                  tunnel: [w2097 _] -> w2085
                  tunnel: [w2096 w2102] -> w2079
                  tunnel: w2078 -> [_ w2102]
                  tunnel: w2077 -> [_ _]
                  frame False {
                    n856 = global read "Position_Micos.vi" "Position(Micos)"() -> (w2093:dbl[])
                    n857 = global read "Position_ESP300.vi" "Position_ESP"() -> (w2094:dbl[])
                    n858 = Unbundle(w2101) -> (w2100:dbl[])  [unwired: 1 out]
                    n859 = local read "Signal Segment"() -> (w2099:T3)
                    n860 = Insert Into Array(array=w2093, new element=w2094) -> (w2095:dbl[])  [unwired: 1 in]
                    n861 = Bundle By Name(cluster=w2099, "Spectrum"=w2100, "Position"=w2095) -> (w2098:T3)
                    n862 = call "WriteTextFile.vi"("Signal Segment"=w2098, "Filename"=w2096) -> ("error out"=w2097:errorcluster)  [unwired: 9 in]
                  }
                  frame True {
                  }
                }
                n863 = feedback-in #7(w2079) -> ()
              }
            }
            n864 = property on="Snap" class="Bool (strict)"(error in=w2073, "Value"=FALSE ("Save Once")) -> ()  [unwired: 1 in, 2 out]
          }
          event Value Change {
            n865 = event-data() -> ("NewVal"=w2107:T2)  [unwired: 1 in]
            n866 = Unbundle By Name(w2106) -> ("WriterCtrl"=w2105:refnum<queue>)
            n867 = Bundle By Name(cluster=T68 {"State"=enum."ChangeFormat", "Params"=variant} ("element"), "Params"=w2107) -> (w2109:T68)
            n868 = property on="Record" class="Bool (strict)"("Value"=FALSE ("Save Multiple")) -> (error out=w2104:errorcluster)  [unwired: 2 in, 1 out]
            n869 = Enqueue Element(queue=w2105, element=w2109, error in (no error)=w2104) -> ()  [unwired: 1 in, 3 out]
          }
          event Value Change {
            n870 = event-data() -> ()  [unwired: 1 in, 1 out]
            n871 = case shown="4294966296" "Gain (Voltage Range)" {
              selector: "Gain (Voltage Range)" -> [w2117 _ _ _]
              tunnel: [w2117 w2120 w2123 w2126] -> w2113
              tunnel: [0 ("Value (Signaling)") -180 ("Value (Signaling)") 180 ("Value (Signaling)") -400 ("Value (Signaling)")] -> w2114
              tunnel: [0.0 ("Value (Signaling)") 0.0175 ("Value (Signaling)") 0.0175 ("Value (Signaling)") 0.0055 ("Value (Signaling)")] -> w2115
              frame 100, 200, 400, 1000, 2000, 5000, 10000, Default {
              }
              frame -400 {
                w2120 = T10 400 items=["-100~900 mV"=4294966296, "-20~380 mV"=4294966896, "+/-5 V"=10000, "+/-2 V"=4000, "+/-1 V"=2000, "+/-500 mV"=1000, "+/-200 mV"=400, "+/-100 mV"=200, "+/-50 mV"=100] ("Gain (Voltage Range)")
                # "400mV range, 180 mV offset"
              }
              frame -401 {
                w2123 = T10 400 items=["-100~900 mV"=4294966296, "-20~380 mV"=4294966896, "+/-5 V"=10000, "+/-2 V"=4000, "+/-1 V"=2000, "+/-500 mV"=1000, "+/-200 mV"=400, "+/-100 mV"=200, "+/-50 mV"=100] ("Gain (Voltage Range)")
                # "400mV range, -180 mV offset"
              }
              frame -1000 {
                w2126 = T10 1000 items=["-100~900 mV"=4294966296, "-20~380 mV"=4294966896, "+/-5 V"=10000, "+/-2 V"=4000, "+/-1 V"=2000, "+/-500 mV"=1000, "+/-200 mV"=400, "+/-100 mV"=200, "+/-50 mV"=100] ("Gain (Voltage Range)")
                # "1000mV range, 400 mV offset"
              }
            }
            n872 = property on="Range" class="DigNum (strict)"("Value"=w2113) -> (error out=w2112:errorcluster)  [unwired: 2 in, 1 out]
            n873 = property on="ZeroOffsetCorrection" class="DigNum (strict)"("Val(Sgnl)"=w2115) -> ()  [unwired: 2 in, 2 out]
            n874 = property on="DC Offset" class="DigNum (strict)"(error in=w2112, "Val(Sgnl)"=w2114) -> ()  [unwired: 1 in, 2 out]
          }
          event Value Change {
            n875 = event-data() -> ()  [unwired: 1 in, 1 out]
            n876 = property on="Sample Rate" class="DigNum (strict)"("Val(Sgnl)"="SampleRate") -> ()  [unwired: 2 in, 2 out]
          }
          event Value Change {
            w2136 = T11 65280.0 items=["256K"=262144.0, "128K"=131072.0, "64K"=65280.0, "32K"=32768.0, "16K"=16384.0, "8K"=8192.0, "1K"=1024.0, "512"=512.0] ("y")
            n877 = event-data() -> ()  [unwired: 1 in, 1 out]
            n878 = control-ref of="Gage_Config"() -> (w2135:refnum<vi>)
            n879 = property class="Clust (strict)"(reference=w2135) -> (reference out=w2133:refnum<vi>, "Value"=w2134:T19)  [unwired: 1 in, 1 out]
            n880 = Greater? "For HwAverage"(x="Spectrum Length", y=w2136) -> ()  [unwired: 1 out]
            n881 = Bundle By Name(cluster=w2134, "Acquisition.Depth"="Spectrum Length", "Acquisition.Segment Size"="Spectrum Length") -> (w2132:T19)
            n882 = property class="Clust (strict)"(reference=w2133, "Val(Sgnl)"=w2132) -> ()  [unwired: 1 in, 2 out]
          }
          event "Scale(A)_X", "Scale(B)_X": Value Change {
            n883 = event-data() -> ()  [unwired: 1 in, 1 out]
            n884 = control-ref of="Graph (A)"() -> (w2141:refnum<vi>)
            n885 = control-ref of="Graph (B)"() -> (w2140:refnum<vi>)
            n886 = Build Array("Scale(A)_X", "Scale(B)_X") -> (w2142:bool[])
            n887 = Build Array(w2141, w2140) -> (w2139:refnum<vi>[])
            n888 = for {
              tunnel: w2142 -> [w2146] mode=indexing
              tunnel: w2139 -> [w2145] mode=indexing
              n889 = case shown="True" w2146 {
                tunnel: w2145 -> [_ w2149]
                frame False {
                }
                frame True {
                  n890 = property class="XYGraph (strict)"(reference=w2149) -> (reference out=w2147:refnum<vi>, "Value"=w2148:cluster{dbl[], dbl[]})  [unwired: 1 in, 1 out]
                  n891 = Unbundle(w2148) -> (w2157:dbl[])  [unwired: 1 out]
                  n892 = Array Size(array=w2157) -> (size(s)=w2155:i32)
                  n893 = Decrement(x=w2155) -> (x-1=w2156:i32)
                  n894 = Array Max & Min(array=w2157) -> (max value=w2152:dbl, min value=w2159:dbl)  [unwired: 2 out]
                  n895 = Index Array(array=w2157, index #1=0 ("index"), index #2=w2156) -> (element #2=w2153:dbl)  [unwired: 1 out]
                  n896 = In Range and Coerce(upper limit=w2152, x=0.0, lower limit=w2159) -> (coerced(x)=w2160:dbl)  [unwired: 1 out]
                  n897 = Round To Nearest(number=w2153) -> (nearest integer value=w2151:dbl)
                  n898 = Round Toward -Infinity(1:w2160) -> (0:w2150:dbl)
                  n899 = property on="Property Node" class="XYGraph (strict)"(reference=w2147, "XScale.Maximum"=w2151, "XScale.Minimum"=w2150) -> ()  [unwired: 1 in, 2 out]
                }
              }
            }
          }
          event "Scale(B)_Y", "Scale(A)_Y": Value Change {
            n900 = event-data() -> ()  [unwired: 1 in, 1 out]
            n901 = control-ref of="Graph (A)"() -> (w2167:refnum<vi>)
            n902 = control-ref of="Graph (B)"() -> (w2166:refnum<vi>)
            n903 = Build Array("Scale(A)_Y", "Scale(B)_Y") -> (w2163:bool[])
            n904 = Build Array(w2167, w2166) -> (w2162:refnum<vi>[])
            n905 = for {
              tunnel: w2163 -> [w2169] mode=indexing
              tunnel: w2162 -> [w2168] mode=indexing
              n906 = case shown="True" w2169 {
                tunnel: w2168 -> [_ w2170]
                frame False {
                }
                frame True {
                  n907 = call-poly "Autoscale_Y.vi"("GraphRef"=w2170) -> ()  [unwired: 11 in]
                }
              }
            }
          }
          event "Scale(A)X--", "Scale(A)X++", "Scale(B)X--", "Scale(B)X++": Value Change {
            w2172 = dbl[] [0.25, 1.0, 0.25, 1.0]  # ZoomIn/OutSetting
            n908 = event-data() -> ()  [unwired: 1 in, 1 out]
            n909 = control-ref of="Graph (A)"() -> (w2180:refnum<vi>)
            n910 = control-ref of="Graph (B)"() -> (w2179:refnum<vi>)
            n911 = Build Array("Scale(A)X++", "Scale(A)X--", "Scale(B)X++", "Scale(B)X--") -> (w2173:bool[])
            n912 = Build Array(w2180, w2180, w2179, w2179) -> (w2178:refnum<vi>[])
            n913 = for {
              tunnel: w2178 -> [w2183] mode=indexing
              tunnel: w2173 -> [w2182] mode=indexing
              tunnel: w2172 -> [w2181] mode=indexing
              n914 = case shown="True" w2182 {
                tunnel: w2183 -> [_ w2185]
                tunnel: w2181 -> [_ w2184]
                frame False {
                }
                frame True {
                  # "Zoom In"
                  n915 = property on="Property Node" class="XYGraph (strict)"(reference=w2185) -> (reference out=w2186:refnum<vi>, "XScale.Maximum"=w2195:dbl, "XScale.Minimum"=w2194:dbl)  [unwired: 1 in, 1 out]
                  n916 = Add(x=w2195, y=w2194) -> (x+y=w2193:dbl)
                  n917 = Subtract(x=w2195, y=w2194) -> (x-y=w2191:dbl)
                  n918 = Multiply(x=0.5, y=w2193) -> (x*y=w2190:dbl)
                  n919 = Multiply(x=w2191, y=w2184) -> (x*y=w2189:dbl)
                  n920 = Add(x=w2190, y=w2189) -> (x+y=w2188:dbl)
                  n921 = Subtract(x=w2190, y=w2189) -> (x-y=w2187:dbl)
                  n922 = property on="Property Node" class="XYGraph (strict)"(reference=w2186, "XScale.Maximum"=w2188, "XScale.Minimum"=w2187) -> ()  [unwired: 1 in, 2 out]
                }
              }
            }
          }
          event "Scale(A)Y++", "Scale(A)Y--", "Scale(B)Y++", "Scale(B)Y--": Value Change {
            n923 = event-data() -> ()  [unwired: 1 in, 1 out]
            n924 = control-ref of="Graph (A)"() -> (w2205:refnum<vi>)
            n925 = control-ref of="Graph (B)"() -> (w2204:refnum<vi>)
            n926 = Build Array(w2205, w2205, w2204, w2204) -> (w2197:refnum<vi>[])
            n927 = Build Array("Scale(A)Y++", "Scale(A)Y--", "Scale(B)Y++", "Scale(B)Y--") -> (w2199:bool[])
            n928 = for {
              tunnel: w2199 -> [w2208] mode=indexing
              tunnel: dbl[] [0.5, 2.0, 0.5, 2.0] -> [w2207] mode=indexing
              tunnel: w2197 -> [w2206] mode=indexing
              n929 = case shown="True" w2208 {
                tunnel: w2207 -> [_ w2210]
                tunnel: w2206 -> [_ w2209]
                frame False {
                }
                frame True {
                  n930 = call "Y_Scale_Change.vi"("Ratio"=w2210, "GraphRef"=w2209) -> ()  [unwired: 10 in]
                }
              }
            }
          }
          event User Event {
            n931 = event-data() -> ("Command"=w2212:T91, "Params."=w2232:variant)  [unwired: 1 in]
            n932 = Variant To Data(type=cluster{"Horizontal(%)":dbl, "Vertical(%)":dbl} {"Horizontal(%)"=0.0, "Vertical(%)"=0.0}, Variant=w2232) -> (data=w2230:cluster{"Horizontal(%)":dbl, "Vertical(%)":dbl})  [unwired: 1 in, 1 out]
            n933 = Unbundle By Name(w2230) -> ("Horizontal(%)"=w2221:dbl, "Vertical(%)"=w2220:dbl)
            n934 = control-ref of="Destination"() -> (w2227:refnum<vi>)
            n935 = call-poly <vilib>:"Array To Matrix.vi"("Real 2D Array"=dbl[][] [[5.0, 0.0, 1.0], [0.0, 5.0, 1.0], [0.0, 0.0, 1.0]]) -> ("Real Matrix"=w2217:T92)
            n936 = Build Array(w2221, w2220, 1.0 ("element")) -> (w2216:dbl[])
            n937 = property on="Property Node" class="Arr (strict)"(reference=w2227) -> (reference out=w2229:refnum<vi>, error out=w2228:errorcluster, "Value"=w2226:dbl[])  [unwired: 1 in]
            n938 = call-poly <vilib>:"A x B.vi"("Vector"=w2216, "A"=w2217) -> ("A x Vector"=w2215:dbl[])  [unwired: 1 out]
            n939 = Index Array(array=w2215) -> (element #1=w2214:dbl, element #2=w2213:dbl)  [unwired: 2 in]
            n940 = control-ref of="MoveAbs(Micos)"() -> (w2211:refnum<vi>)
            n941 = in-place {
              in-place-border: w2214 -> [w2243]
              in-place-border: w2213 -> [w2242]
              n942 = in-place-array #8(w2226, 0, 1) -> ()  [unwired: 2 out]
              n943 = in-place-array #8(w2243, w2242) -> (w2225:dbl[])  [unwired: 2 out]
            }
            n944 = case shown="\"MouseDoubleClick\"" w2212 {
              tunnel: w2229 -> [_ w2238 w2241]
              tunnel: w2228 -> [_ w2237 w2240]
              tunnel: w2225 -> [_ w2236 w2239]
              tunnel: w2211 -> [_ w2235 _]
              frame Default {
              }
              frame "MouseDoubleClick" {
                n945 = property on="Property Node" class="Arr (strict)"(reference=w2238, error in=w2237, "Value"=w2236) -> (error out=w2234:errorcluster)  [unwired: 1 out]
                n946 = property on="Property Node" class="Bool (strict)"(reference=w2235, error in=w2234, "Val(Sgnl)"=TRUE ("Value")) -> ()  [unwired: 2 out]
              }
              frame "MouseClick" {
                n947 = property on="Property Node" class="Arr (strict)"(reference=w2241, error in=w2240, "Value"=w2239) -> ()  [unwired: 2 out]
              }
            }
          }
          event "CameraOn": Value Change {
            n948 = event-data() -> ()  [unwired: 1 in, 1 out]
            n949 = disable-structure shown="IMAQdx_EXIST==TRUE" {
              disable-tunnel: w2245 -> [w2247 _]
              frame condition #0 {
                n950 = vi-ref "GenericCameraCore.vi"() -> (w2252:refnum<vi>)
                n951 = property class="VI Interface Type 2"(reference=w2252) -> (reference out=w2251:refnum<vi>, "Path"=w2250:path)  [unwired: 1 in, 1 out]
                n952 = Open VI Reference(type specifier VI Refnum (for type only)=w2251, vi path=w2250, options=128) -> (vi reference=w2249:refnum<vi>)  [unwired: 3 in, 1 out]
                n953 = call-by-ref "Start Asynchronous Call"(reference=w2249, "CameraEvent"=w2247, "Camera Selector"=T87 "cam0") -> ()  [unwired: 11 in, 2 out]
              }
              frame condition #1 (active) {
              }
            }
          }
        }
      }
      n954 = case "Main Data Acquisition Device Selector" shown="\"AnalogDisc\"" w176 {
        tunnel: w270 -> [w411 w460 w474 _ _]
        tunnel: w162 -> [w412 w461 w473 _ _]
        tunnel: w262 -> [w413 w462 w475 _ _]
        tunnel: [w410 w459 w472 _ _] -> w165
        frame "Gage" {
          # "Gage"
          n955 = disable-structure shown="GAGE_EXIST==TRUE" {
            disable-tunnel: w412 -> [w434 _]
            disable-tunnel: w411 -> [w433 _]
            disable-tunnel: [w426 _] -> w410
            frame condition #0 (active) {
              n956 = property on="Gage_Config" class="Clust (strict)"() -> ("Value"=w418:T19)  [unwired: 2 in, 2 out]
              n957 = vi-ref "SecondaryData_Position.vi"() -> (w423:refnum<vi>)
              n958 = Bundle By Name(cluster=T72 {"SecondaryDataVIRef."=refnum, "Option"=0} ("SecondaryDataParams."), "SecondaryDataVIRef."=w423, "Option"=0) -> (w425:T72)
              n959 = Bundle By Name(cluster=T60 {"DWF States"=enum."SetAll_AcquChTrig_", "Variant"=variant} ("element"), "Variant"=w418) -> (w419:T60)
              n960 = Bundle By Name(cluster=T60 {"DWF States"=enum."SetSecondaryDataRef._", "Variant"=variant} ("element"), "Variant"=w425) -> (w420:T60)
              n961 = Build Array(T60 {"DWF States"=enum."Enumerate", "Variant"=variant} ("element"), T60 {"DWF States"=enum."Open", "Variant"=variant} ("element"), w420, w419) -> (w429:T60[])
              n962 = for {
                shift-right: [w438] -> w430
                shift-left: w433 -> [w439]
                tunnel: w429 -> [w437] mode=indexing
                shift-right: [w436] -> w416
                shift-left: _ -> [w435]
                n963 = Enqueue Element(queue=w439, element=w437, error in (no error)=w435) -> (queue out=w438:refnum<queue>, error out=w436:errorcluster)  [unwired: 1 in, 1 out]
              }
              n964 = control-ref of="Gage_Config"() -> (w428:refnum<vi>)
              n965 = property on="Get Some Values update" class="Clust (strict)"(reference=w428, error in=w416, "Val(Sgnl)"=w418) -> (error out=w427:errorcluster)  [unwired: 1 out]
              n966 = call <instrlib>:"Gage_Core.vi"("error in"=w427, "SignalBufferQueue"=w434, "DWFCtrlQueue in"=w430) -> ("error out"=w415:errorcluster)  [unwired: 8 in]
              n967 = Release Queue(queue=w430, error in (no error)=w415) -> (error out=w426:errorcluster)  [unwired: 1 in, 2 out]
            }
            frame condition #1 {
            }
          }
          n968 = Unbundle By Name(w413) -> ("Graph"=w414:T67[])
          n969 = for {
            tunnel: w414 -> [w441] mode=indexing
            n970 = Unbundle By Name(w441) -> ("XY_Graph"=w440:refnum<vi>)
            n971 = property class="XYGraph (strict)"(reference=w440, "YScale.FormatString"="%#_3pV" ("Y Scale.Format String")) -> ()  [unwired: 1 in, 2 out]
          }
        }
        frame "KnifeEdge_Emu", "FakeSignal(Emulator)" {
          # "Beam profile:\nfocus at [0.5,0.5,0.5]\n\n3D Image Center:\n[0.5, 0.5, 1.5]\nZ range: 1.01 -1.99"
          # "Emulate Signal for testing. (Beam Profile and Image)"
          n972 = Unbundle By Name(w462) -> ("Graph"=w463:T67[])
          n973 = vi-ref "SecondaryData_Position.vi"() -> (w452:refnum<vi>)
          n974 = for {
            tunnel: w463 -> [w470] mode=indexing
            n975 = Unbundle By Name(w470) -> ("XY_Graph"=w469:refnum<vi>)
            n976 = property class="XYGraph (strict)"(reference=w469, "YScale.FormatString"="%#_3pV" ("Y Scale.Format String")) -> ()  [unwired: 1 in, 2 out]
          }
          n977 = Bundle By Name(cluster=T72 {"SecondaryDataVIRef."=refnum, "Option"=0} ("SecondaryDataParams."), "SecondaryDataVIRef."=w452, "Option"=0) -> (w454:T72)
          n978 = Bundle By Name(cluster=T60 {"DWF States"=enum."SetAll_AcquChTrig_", "Variant"=variant} ("element"), "Variant"="GenericDAQ_Config") -> (w444:T60)
          n979 = Bundle By Name(cluster=T60 {"DWF States"=enum."SetSecondaryDataRef._", "Variant"=variant} ("element"), "Variant"=w454) -> (w449:T60)
          n980 = Build Array(T60 {"DWF States"=enum."Enumerate", "Variant"=variant} ("element"), T60 {"DWF States"=enum."Open", "Variant"=variant} ("element"), w449, w444) -> (w455:T60[])
          n981 = for {
            shift-right: [w467] -> w456
            shift-left: w460 -> [w468]
            tunnel: w455 -> [w466] mode=indexing
            shift-right: [w465] -> w445
            shift-left: _ -> [w464]
            n982 = Enqueue Element(queue=w468, element=w466, error in (no error)=w464) -> (queue out=w467:refnum<queue>, error out=w465:errorcluster)  [unwired: 1 in, 1 out]
          }
          n983 = property on="GenericDAQ_Config" class="Clust (strict)"(error in=w445, "Val(Sgnl)"="GenericDAQ_Config") -> (error out=w446:errorcluster)  [unwired: 1 in, 1 out]
          n984 = call <instrlib>:"GenericDAQCore.vi"("error in"=w446, "SignalBufferQueue"=w461, "DWFCtrlQueue in"=w456) -> ("error out"=w447:errorcluster)  [unwired: 8 in]
          n985 = Release Queue(queue=w456, error in (no error)=w447) -> (error out=w459:errorcluster)  [unwired: 1 in, 2 out]
        }
        frame "AnalogDisc" {
          # "Gage"
          n986 = disable-structure shown="AD_EXIST==TRUE" {
            disable-tunnel: w474 -> [w500 _]
            disable-tunnel: w473 -> [w492 _]
            disable-tunnel: [w482 _] -> w472
            frame condition #0 {
              n987 = property on="AnalogDisc_Configs" class="Clust (strict)"() -> ("Value"=w479:T20)  [unwired: 2 in, 2 out]
              n988 = vi-ref "SecondaryData_Position.vi"() -> (w486:refnum<vi>)
              n989 = Bundle By Name(cluster=T73 {"SecondaryDataVIRef."=refnum, "Option"=0} ("SecondaryDataParams."), "SecondaryDataVIRef."=w486, "Option"=0) -> (w484:T73)
              n990 = Bundle By Name(cluster=T60 {"DWF States"=enum."SetMode_", "Variant"=variant} ("element"), "Variant"=enum16{"Normal", "Turbo"}."Turbo" ("Mode")) -> (w495:T60)
              n991 = Bundle By Name(cluster=T60 {"DWF States"=enum."SetAll_AcquChTrig_", "Variant"=variant} ("element"), "Variant"=w479) -> (w497:T60)
              n992 = Bundle By Name(cluster=T60 {"DWF States"=enum."SetSecondaryDataRef._", "Variant"=variant} ("element"), "Variant"=w484) -> (w480:T60)
              n993 = Build Array(T60 {"DWF States"=enum."CloseAll", "Variant"=variant} ("element"), T60 {"DWF States"=enum."Open", "Variant"=variant} ("element"), w497, T60 {"DWF States"=enum."fConfigurate", "Variant"=variant} ("element"), w495, T60 {"DWF States"=enum."fStart", "Variant"=variant} ("element"), w480) -> (w493:T60[])
              n994 = for {
                shift-right: [w506] -> w483
                shift-left: w500 -> [w507]
                tunnel: w493 -> [w505] mode=indexing
                shift-right: [w504] -> w481
                shift-left: errorcluster {"status"=FALSE, "code"=0, "source"=""} ("error out") -> [w503]
                n995 = Enqueue Element(queue=w507, element=w505, error in (no error)=w503) -> (queue out=w506:refnum<queue>, error out=w504:errorcluster)  [unwired: 1 in, 1 out]
              }
              n996 = control-ref of="AnalogDisc_Configs"() -> (w490:refnum<vi>)
              n997 = property class="Clust (strict)"(reference=w490, error in=w481, "Val(Sgnl)"=w479) -> (error out=w491:errorcluster)  [unwired: 1 out]
              n998 = call <instrlib>:"AnalogDisc_Core.vi"("error in"=w491, "SignalBufferQueue"=w492, "DWFCtrlQueue in"=w483) -> ("error out"=w477:errorcluster)  [unwired: 6 in, 2 out]
              n999 = Release Queue(queue=w483, error in (no error)=w477) -> (error out=w482:errorcluster)  [unwired: 1 in, 2 out]
            }
            frame condition #1 (active) {
            }
          }
          n1000 = Unbundle By Name(w475) -> ("Graph"=w476:T67[])
          n1001 = for {
            tunnel: w476 -> [w509] mode=indexing
            n1002 = Unbundle By Name(w509) -> ("XY_Graph"=w508:refnum<vi>)
            n1003 = property class="XYGraph (strict)"(reference=w508, "YScale.FormatString"="%#_3pV" ("Y Scale.Format String")) -> ()  [unwired: 1 in, 2 out]
          }
        }
        frame Default {
        }
        frame "None" {
        }
      }
      n1004 = while "subApps Loop" {
        shift-right: [w522] -> w230
        shift-left: w351 -> [w529]
        tunnel: w269 -> [w538]
        tunnel: w263 -> [w518]
        tunnel: w158 -> [w519]
        stop <- w537 stop-if-true
        n1005 = Unbundle By Name(w518) -> ("InfoRef"=w527:refnum<vi>, "AppsLock"=w525:T63)
        n1006 = Unbundle By Name(w518) -> ("LaserCtrlMethod"=w520:T17)
        n1007 = property class="Str"(reference=w527, error in=w529, "Value"="subProgram Ready...") -> (error out=w530:errorcluster)  [unwired: 1 out]
        n1008 = Dequeue Element(queue=w538, error in (no error)=w530) -> (queue out=w532:refnum<queue>, element=w534:T71, timed out?=w535:bool, error out=w517:errorcluster)  [unwired: 1 in]
        n1009 = case shown="\"SDG_II\"" w520 {
          tunnel: [w541 w544 w547] -> w521
          tunnel: w517 -> [w539 w542 w546]
          tunnel: [w540 w543 w545] -> w516
          frame "BNC" {
            n1010 = property on="Rep.Rate (BNC)" class="DigNum (strict)"(error in=w539) -> (error out=w540:errorcluster, "Value"=w541:dbl)  [unwired: 1 in, 1 out]
          }
          frame "SRS_DG535" {
            n1011 = property on="Internal/Burst Rate" class="DigNum (strict)"(error in=w542) -> (error out=w543:errorcluster, "Value"=w544:dbl)  [unwired: 1 in, 1 out]
          }
          frame "SDG_II" {
            n1012 = property on="Internal/Burst Rate" class="DigNum (strict)"(error in=w546) -> (error out=w545:errorcluster, "Value"=w547:dbl)  [unwired: 1 in, 1 out]
          }
        }
        n1013 = Select(t=States-AToF."Idle", s=w535, f=w534) -> (s? t:f=w536:T71)
        n1014 = call <vilib>:"Acquire Semaphore.vi"("error in (no error)"=w516, "semaphore"=w525) -> ("error out"=w526:errorcluster, "semaphore out"=w524:T63)  [unwired: 3 in, 1 out]
        n1015 = case shown="\"Imaging_Micos\"" w536 {
          selector: w536 -> [_ _ _ _ _ _ _ _ _ _ _ _ _ _ _ _ _ w1079]
          tunnel: [_ _ _ _ _ _ _ _ _ _ _ _ _ _ _ TRUE _ _] -> w537
          tunnel: w526 -> [_ _ w590 w626 w660 w704 w752 w794 w836 w882 w930 w969 w984 _ _ w1069 _ _]
          tunnel: w532 -> [_ _ w586 w622 w655 w701 w750 w790 w832 w879 w926 _ w981 _ _ w1068 _ _]
          tunnel: [_ _ w589 w625 w659 w703 w755 w793 w835 w881 w929 w966 w983 _ _ _ _ _] -> w531
          tunnel: w518 -> [w564 w581 w587 w623 w657 w692 w748 w791 w833 w880 w927 w974 w979 _ w1024 w1058 _ _]
          tunnel: w527 -> [_ _ _ _ _ _ _ _ _ _ _ _ _ _ _ _ _ w1072]
          tunnel: w521 -> [_ _ w584 w620 w654 w691 w740 w787 w829 w872 w923 _ w975 _ _ _ _ _]
          tunnel: w519 -> [_ _ w583 w619 _ _ w739 _ _ _ _ _ _ w1013 _ _ _ _]
          frame "Initialize" {
            n1016 = Unbundle By Name(w564) -> ("Micos"=w554:refnum<queue>, "WriterCtrl"=w563:refnum<queue>)
            n1017 = disable-structure shown="Disabled" {
              frame Disabled {
                n1018 = control-ref of="Gain (Voltage Range)"() -> ()  [unwired: 1 out]
                n1019 = control-ref of="Spectrum Length"() -> ()  [unwired: 1 out]
                n1020 = control-ref of="SampleRate"() -> ()  [unwired: 1 out]
                n1021 = control-ref of="Processing Mode\nNot Needed"() -> ()  [unwired: 1 out]
              }
              frame Enabled {
              }
            }
            n1022 = local read "Files Format"() -> (w565:T2)
            n1023 = Bundle By Name(cluster=T68 {"State"=enum."ChangeFormat", "Params"=variant} ("element"), "Params"=w565) -> (w566:T68)
            n1024 = Enqueue Element(queue=w563, element=w566) -> ()  [unwired: 2 in, 3 out]
            n1025 = Bundle By Name(cluster=T74 {"State"=enum."MotorEnable(1)", "Params."=variant} ("element"), "Params."=TRUE) -> (w556:T74)
            n1026 = Enqueue Element(queue=w554, element=w556) -> ()  [unwired: 2 in, 3 out]
            n1027 = control-ref of="Set Mode"() -> ()  [unwired: 1 out]
            n1028 = control-ref of="Velocity(Micos)"() -> (w562:refnum<vi>)
            n1029 = control-ref of="Accele.(Micos)"() -> (w560:refnum<vi>)
            n1030 = control-ref of="Velocity (ESP)"() -> (w559:refnum<vi>)
            n1031 = control-ref of="Accele. (ESP)"() -> (w553:refnum<vi>)
            n1032 = control-ref of="ZeroOffsetCorrection"() -> (w558:refnum<vi>)
            n1033 = control-ref of="Delay(LDI-Rej.)"() -> (w552:refnum<vi>)
            n1034 = control-ref of="Delay(PI)"() -> (w550:refnum<vi>)
            n1035 = control-ref of="Internal/Burst Rate"() -> (w551:refnum<vi>)
            n1036 = control-ref of="Trigger Mode (SRS)"() -> (w548:refnum<vi>)
            n1037 = Build Array(w562, w560, w559, w553, w558, w551, w552, w550) -> (w561:refnum<vi>[])
            n1038 = disable-structure "Diagram Disable Structure" shown="Enabled" {
              frame Enabled {
                # "Initial Values for SaveOnce function"
                n1039 = control-ref of="Cali."() -> (w573:refnum<vi>)
                n1040 = property on="This has to be enabled. No idea why." class="Arr (strict)"(reference=w573) -> (reference out=w572:refnum<vi>, error out=w574:errorcluster, "Value"=w575:dbl[])  [unwired: 1 in]
                n1041 = property on="Property Node" class="Arr (strict)"(reference=w572, error in=w574, "Val(Sgnl)"=w575) -> ()  [unwired: 2 out]
              }
              frame Disabled {
              }
            }
            n1042 = Build Array(w548) -> (w549:refnum<vi>[])
            n1043 = for {
              tunnel: w561 -> [w577] mode=indexing
              n1044 = property on="Property Node" class="DigNum (strict)"(reference=w577) -> (reference out=w576:refnum<vi>, error out=w579:errorcluster, "Value"=w578:dbl)  [unwired: 1 in]
              n1045 = property on="Property Node" class="DigNum (strict)"(reference=w576, error in=w579, "Val(Sgnl)"=w578) -> ()  [unwired: 2 out]
            }
            n1046 = for {
              tunnel: w549 -> [w569] mode=indexing
              n1047 = property on="Property Node" class="Enum (strict)"(reference=w569) -> (reference out=w568:refnum<vi>, error out=w571:errorcluster, "Value"=w570:T7)  [unwired: 1 in]
              n1048 = property on="Property Node" class="Enum (strict)"(reference=w568, error in=w571, "Val(Sgnl)"=w570) -> ()  [unwired: 2 out]
            }
          }
          frame "CalcMzArray" {
            # "data processing need separate contrl + data queue"
            n1049 = Unbundle By Name(w581) -> ("ProcCore_CtrlQueue"=w580:refnum<queue>)
            n1050 = Enqueue Element(queue=w580, element=T75 {"Command"=enum."CalcMzArray", "Params"=variant}) -> ()  [unwired: 2 in, 3 out]
          }
          frame "Meander_MCS" {
            n1051 = global read "Position_Micos.vi" "Position(Micos)"() -> (w585:dbl[])
            n1052 = call "CreateMeanderMask_3d.vi"("Rep. Rate (Hz)"=w584, "Start Position"=w585) -> ("Laser_Ctrl"=w591:bool, "start/end points"=w592:cluster{dbl, dbl, dbl}[][], "Canceled"=w593:bool, "ImageParameter"=w588:T93)  [unwired: 6 in]
            n1053 = case shown="False" w593 {
              tunnel: w592 -> [w617 _]
              tunnel: w590 -> [w604 w618]
              tunnel: w591 -> [w616 _]
              tunnel: [w607 w618] -> w589
              tunnel: w588 -> [w600 _]
              tunnel: w587 -> [w602 _]
              tunnel: w586 -> [w601 _]
              tunnel: w583 -> [w596 _]
              frame False {
                n1054 = Unbundle By Name(w596) -> ()  [unwired: 1 out]
                n1055 = Unbundle By Name(w600) -> ("Start Position"=w610:dbl[], "StepWidth"=w609:dbl[], "Dimension"=w608:i32[], "ScanSpeed"=w598:dbl)
                n1056 = property on="Depth" class="DigNum (strict)"() -> ("Value"=w599:dbl)  [unwired: 2 in, 2 out]
                n1057 = control-ref of="Velocity(Micos)"() -> (w595:refnum<vi>)
                n1058 = Bundle By Name(cluster=T77 {"Start Position"=[], "StepWidth"=[], "Dimension"=[], "SpecLength"=0} ("File Header"), "SpecLength"=w599, "Start Position"=w610, "StepWidth"=w609, "Dimension"=w608) -> (w611:T77)
                n1059 = Unbundle By Name(w602) -> ("Micos"=w597:refnum<queue>, "WriterCtrl"=w603:refnum<queue>)
                n1060 = Bundle By Name(cluster=T68 {"State"=enum."SetHeader", "Params"=variant} ("element"), "Params"=w611) -> (w613:T68)
                n1061 = property class="DigNum (strict)"(reference=w595) -> ("Value"=w594:dbl)  [unwired: 1 in, 2 out]
                n1062 = Enqueue Element(queue=w603, element=w613, error in (no error)=w604) -> (error out=w605:errorcluster)  [unwired: 1 in, 2 out]
                n1063 = call "MeanderCtrl_3d_StageRefs.vi"("QueuesRef"=w602, "MotionStageRefs"=w597, "AppsRef"=w601, "start/end points"=w617, "Laser_Ctrl"=w616, "error in"=w605, "HighSpeed"=w594, "ScanSpeed"=w598) -> ("error out"=w606:errorcluster)  [unwired: 5 in, 2 out]
                n1064 = property on="Record" class="Bool (strict)"(error in=w606, "Val(Sgnl)"=FALSE) -> (error out=w607:errorcluster)  [unwired: 1 in, 1 out]
              }
              frame True {
              }
            }
          }
          frame "CleanSurface" {
            n1065 = global read "Position_Micos.vi" "Position(Micos)"() -> (w621:dbl[])
            n1066 = call "CleanSurface_3d.vi"("Rep. Rate (Hz)"=w620, "Start Position"=w621) -> ("BNC_Ctrl"=w627:bool, "start/end points"=w628:cluster{dbl, dbl, dbl}[][], "Canceled"=w629:bool, "ImageParameter"=w624:T94)  [unwired: 6 in]
            n1067 = case shown="False" w629 {
              tunnel: w628 -> [w652 _]
              tunnel: w626 -> [w639 w653]
              tunnel: w627 -> [w651 _]
              tunnel: [w642 w653] -> w625
              tunnel: w624 -> [w632 _]
              tunnel: w623 -> [w636 _]
              tunnel: w622 -> [w635 _]
              tunnel: w619 -> [_ _]
              frame False {
                n1068 = Unbundle By Name(w636) -> ("WriterCtrl"=w637:refnum<queue>)
                n1069 = Unbundle By Name(w632) -> ("MeanderSpeed"=w630:dbl, "Start Position"=w645:dbl[], "StepWidth"=w644:dbl[], "Dimension"=w643:i32[])
                n1070 = property on="Depth" class="DigNum (strict)"() -> ("Value"=w631:dbl)  [unwired: 2 in, 2 out]
                n1071 = Bundle By Name(cluster=T77 {"Start Position"=[], "StepWidth"=[], "Dimension"=[], "SpecLength"=0} ("File Header"), "Start Position"=w645, "StepWidth"=w644, "Dimension"=w643, "SpecLength"=w631) -> (w646:T77)
                n1072 = control-ref of="Velocity(Micos)"() -> (w634:refnum<vi>)
                n1073 = Bundle By Name(cluster=T68 {"State"=enum."SetHeader", "Params"=variant} ("element"), "Params"=w646) -> (w648:T68)
                n1074 = property class="DigNum (strict)"(reference=w634) -> ("Value"=w633:dbl)  [unwired: 1 in, 2 out]
                n1075 = Enqueue Element(queue=w637, element=w648, error in (no error)=w639) -> (error out=w640:errorcluster)  [unwired: 1 in, 2 out]
                n1076 = Unbundle By Name(w636) -> ("Micos"=w638:refnum<queue>)
                n1077 = call "MeanderCtrl_3d_StageRefs.vi"("QueuesRef"=w636, "MotionStageRefs"=w638, "AppsRef"=w635, "start/end points"=w652, "Laser_Ctrl"=w651, "error in"=w640, "HighSpeed"=w633, "ScanSpeed"=w630) -> ("error out"=w641:errorcluster)  [unwired: 5 in, 2 out]
                n1078 = property on="Record" class="Bool (strict)"(error in=w641, "Val(Sgnl)"=FALSE) -> (error out=w642:errorcluster)  [unwired: 1 in, 1 out]
              }
              frame True {
              }
            }
          }
          frame "Meander_Npt" {
            n1079 = global read "Position_ESP300.vi" "Position_ESP"() -> (w656:dbl[])
            n1080 = call "CreateMeanderMask_3d.vi"("Rep. Rate (Hz)"=w654, "Start Position"=w656) -> ("Laser_Ctrl"=w661:bool, "start/end points"=w663:cluster{dbl, dbl, dbl}[][], "Canceled"=w664:bool, "ImageParameter"=w658:T93)  [unwired: 6 in]
            n1081 = Unbundle By Name(w658) -> ("ScanSpeed"=w662:dbl)
            n1082 = case shown="False" w664 {
              tunnel: w663 -> [w687 _]
              tunnel: w660 -> [w672 w688]
              tunnel: w662 -> [w686 _]
              tunnel: w661 -> [w685 _]
              tunnel: [w675 w688] -> w659
              tunnel: w658 -> [w679 _]
              tunnel: w657 -> [w667 _]
              tunnel: w655 -> [w666 _]
              frame False {
                n1083 = Unbundle By Name(w679) -> ("Start Position"=w678:dbl[], "StepWidth"=w677:dbl[], "Dimension"=w676:i32[])
                n1084 = Unbundle By Name(w667) -> ("WriterCtrl"=w668:refnum<queue>)
                n1085 = property on="Depth" class="DigNum (strict)"() -> ("Value"=w665:dbl)  [unwired: 2 in, 2 out]
                n1086 = Bundle By Name(cluster=T77 {"Start Position"=[], "StepWidth"=[], "Dimension"=[], "SpecLength"=0} ("File Header"), "Start Position"=w678, "StepWidth"=w677, "Dimension"=w676, "SpecLength"=w665) -> (w680:T77)
                n1087 = control-ref of="Velocity (ESP)"() -> (w671:refnum<vi>)
                n1088 = Bundle By Name(cluster=T68 {"State"=enum."SetHeader", "Params"=variant} ("element"), "Params"=w680) -> (w682:T68)
                n1089 = property class="DigNum (strict)"(reference=w671) -> ("Value"=w670:dbl)  [unwired: 1 in, 2 out]
                n1090 = Enqueue Element(queue=w668, element=w682, error in (no error)=w672) -> (error out=w673:errorcluster)  [unwired: 1 in, 2 out]
                n1091 = Unbundle By Name(w667) -> ("ESP300"=w669:refnum<queue>)
                n1092 = call "MeanderCtrl_3d_StageRefs.vi"("QueuesRef"=w667, "MotionStageRefs"=w669, "AppsRef"=w666, "start/end points"=w687, "Laser_Ctrl"=w685, "error in"=w673, "HighSpeed"=w670, "ScanSpeed"=w686) -> ("error out"=w674:errorcluster)  [unwired: 5 in, 2 out]
                n1093 = property on="Record" class="Bool (strict)"(error in=w674, "Val(Sgnl)"=FALSE) -> (error out=w675:errorcluster)  [unwired: 1 in, 1 out]
              }
              frame True {
              }
            }
          }
          frame "KnifeEdgeExpt" {
            n1094 = global read "Position_Micos.vi" "Position(Micos)"() -> (w700:dbl[])
            n1095 = vi-ref "SecondaryData_Position.vi"() -> (w694:refnum<vi>)
            n1096 = Bundle By Name(cluster=T72 {"SecondaryDataVIRef."=refnum, "Option"=0} ("SecondaryDataParams."), "SecondaryDataVIRef."=w694, "Option"=0) -> (w693:T72)
            n1097 = call "KnifeEdgeExpt.vi"("Rep. Rate (Hz)"=w691, "Start Position"=w700) -> ("SDG_Ctrl"=w705:bool, "Canceled"=w707:bool, "Angle_Incident"=w699:dbl, "X/Y (T:Y)"=w698:bool, "ImageParameter"=w702:T94, "w_fit_init."=w690:dbl[], "z0_fit_init."=w689:dbl[])  [unwired: 2 in, 1 out]
            n1098 = Unbundle By Name(w702) -> ("MeanderSpeed"=w706:dbl)
            n1099 = vi-ref "BeamProfile_Proc.vi"() -> (w697:refnum<vi>)
            n1100 = case shown="False" w707 {
              tunnel: w704 -> [w711 w736]
              tunnel: w706 -> [w722 _]
              tunnel: w705 -> [w735 _]
              tunnel: [w732 w736] -> w703
              tunnel: w702 -> [w733 _]
              tunnel: w692 -> [w713 _]
              tunnel: w701 -> [w729 _]
              tunnel: w699 -> [w720 _]
              tunnel: w698 -> [w719 _]
              tunnel: w697 -> [w718 _]
              tunnel: w693 -> [w714 _]
              tunnel: w690 -> [w709 _]
              tunnel: w689 -> [w708 _]
              frame False {
                n1101 = control-ref of="Velocity(Micos)"() -> (w728:refnum<vi>)
                n1102 = Unbundle By Name(w713) -> ("MainDAQCoreQueue"=w717:refnum<queue>)
                n1103 = property class="DigNum (strict)"(reference=w728) -> ("Value"=w721:dbl)  [unwired: 1 in, 2 out]
                n1104 = Bundle By Name(cluster=T60 {"DWF States"=enum."SetSecondaryDataRef._", "Variant"=variant} ("element"), "Variant"=w714) -> (w716:T60)
                n1105 = Enqueue Element(queue=w717, element=w716, error in (no error)=w711) -> (error out=w712:errorcluster)  [unwired: 1 in, 2 out]
                n1106 = Unbundle By Name(w733) -> ("Start Position"=w726:dbl[], "StepWidth"=w725:dbl[], "Dimension"=w724:i32[])
                n1107 = property on="Depth" class="DigNum (strict)"() -> ("Value"=w710:dbl)  [unwired: 2 in, 2 out]
                n1108 = Bundle By Name(cluster=T78 {"File Header"={"Start Position"=[], "StepWidth"=[], "Dimension"=[], "SpecLength"=0}, "w_fit_init."=[], "z0_fit_init."=[], "LowSpeed"=0.0, "HighSpeed"=0.0, "x/y?"=FALSE, "IncidentAngle"=0.0} ("BeamProfiling_Params"), "File Header.SpecLength"=w710, "w_fit_init."=w709, "z0_fit_init."=w708, "File Header.Start Position"=w726, "File Header.StepWidth"=w725, "File Header.Dimension"=w724, "LowSpeed"=w722, "HighSpeed"=w721, "IncidentAngle"=w720, "x/y?"=w719) -> (w723:T78)
                n1109 = Unbundle By Name(w713) -> ("Micos"=w730:refnum<queue>)
                n1110 = call "MeanderCtrl_Dynamic,StageRefs.vi"("QueuesRef"=w713, "MotionStageRefs"=w730, "AppsRef"=w729, "subprog_Ref"=w718, "Params."=w723, "Laser_Ctrl"=w735, "error in"=w712, "HighSpeed"=w721, "LowSpeed"=w722) -> ("error out"=w731:errorcluster)  [unwired: 5 in, 1 out]
                n1111 = property on="Record" class="Bool (strict)"(error in=w731, "Val(Sgnl)"=FALSE) -> (error out=w732:errorcluster)  [unwired: 1 in, 1 out]
              }
              frame True {
              }
            }
          }
          frame "KnifeEdgeExpt_Npt" {
            w743 = 1  # Swap ESP/Micos
            n1112 = global read "Position_ESP300.vi" "Position_ESP"() -> (w756:dbl[])
            n1113 = vi-ref "SecondaryData_Position.vi"() -> (w742:refnum<vi>)
            n1114 = call "KnifeEdgeExpt.vi"("Rep. Rate (Hz)"=w740, "Start Position"=w756) -> ("SDG_Ctrl"=w753:bool, "Canceled"=w751:bool, "Angle_Incident"=w747:dbl, "X/Y (T:Y)"=w746:bool, "ImageParameter"=w749:T94, "w_fit_init."=w738:dbl[], "z0_fit_init."=w737:dbl[])  [unwired: 2 in, 1 out]
            n1115 = Bundle By Name(cluster=T73 {"SecondaryDataVIRef."=refnum, "Option"=0} ("SecondaryDataParams."), "SecondaryDataVIRef."=w742, "Option"=w743) -> (w741:T73)
            n1116 = Unbundle By Name(w749) -> ("MeanderSpeed"=w754:dbl)
            n1117 = vi-ref "BeamProfile_Proc.vi"() -> (w745:refnum<vi>)
            n1118 = case shown="False" w751 {
              tunnel: w752 -> [w764 w786]
              tunnel: w754 -> [w773 _]
              tunnel: w753 -> [w785 _]
              tunnel: [w782 w786] -> w755
              tunnel: w749 -> [w783 _]
              tunnel: w748 -> [w761 _]
              tunnel: w750 -> [w779 _]
              tunnel: w747 -> [w772 _]
              tunnel: w746 -> [w771 _]
              tunnel: w745 -> [w770 _]
              tunnel: w741 -> [w766 _]
              tunnel: w739 -> [w762 _]
              tunnel: w738 -> [w758 _]
              tunnel: w737 -> [w757 _]
              frame False {
                n1119 = Unbundle By Name(w762) -> ()  [unwired: 1 out]
                n1120 = Unbundle By Name(w761) -> ("MainDAQCoreQueue"=w769:refnum<queue>)
                n1121 = Bundle By Name(cluster=T60 {"DWF States"=enum."SetSecondaryDataRef._", "Variant"=variant} ("element"), "Variant"=w766) -> (w767:T60)
                n1122 = control-ref of="Velocity (ESP)"() -> (w760:refnum<vi>)
                n1123 = Enqueue Element(queue=w769, element=w767, error in (no error)=w764) -> (error out=w765:errorcluster)  [unwired: 1 in, 2 out]
                n1124 = property class="DigNum (strict)"(reference=w760) -> ("Value"=w759:dbl)  [unwired: 1 in, 2 out]
                n1125 = Unbundle By Name(w783) -> ("Start Position"=w777:dbl[], "StepWidth"=w776:dbl[], "Dimension"=w775:i32[])
                n1126 = property on="Depth" class="DigNum (strict)"() -> ("Value"=w763:dbl)  [unwired: 2 in, 2 out]
                n1127 = Bundle By Name(cluster=T78 {"File Header"={"Start Position"=[], "StepWidth"=[], "Dimension"=[], "SpecLength"=0}, "w_fit_init."=[], "z0_fit_init."=[], "LowSpeed"=0.0, "HighSpeed"=0.0, "x/y?"=FALSE, "IncidentAngle"=0.0} ("BeamProfiling_Params"), "File Header.Start Position"=w777, "File Header.StepWidth"=w776, "File Header.Dimension"=w775, "File Header.SpecLength"=w763, "LowSpeed"=w773, "HighSpeed"=w759, "x/y?"=w771, "IncidentAngle"=w772, "w_fit_init."=w758, "z0_fit_init."=w757) -> (w774:T78)
                n1128 = Unbundle By Name(w761) -> ("ESP300"=w780:refnum<queue>)
                n1129 = call "MeanderCtrl_Dynamic,StageRefs.vi"("QueuesRef"=w761, "MotionStageRefs"=w780, "AppsRef"=w779, "subprog_Ref"=w770, "Params."=w774, "Laser_Ctrl"=w785, "error in"=w765, "HighSpeed"=w759, "LowSpeed"=w773) -> ("error out"=w781:errorcluster)  [unwired: 5 in, 1 out]
                n1130 = property on="Record" class="Bool (strict)"(error in=w781, "Val(Sgnl)"=FALSE) -> (error out=w782:errorcluster)  [unwired: 1 in, 1 out]
              }
              frame True {
              }
            }
          }
          frame "Imaging_Micos" {
            n1131 = global read "Position_Micos.vi" "Position(Micos)"() -> (w789:dbl[])
            n1132 = vi-ref "Imaging_Proc.vi"() -> (w788:refnum<vi>)
            n1133 = call "CreateMeanderMask_3d.vi"("Rep. Rate (Hz)"=w787, "Start Position"=w789) -> ("Laser_Ctrl"=w795:bool, "Canceled"=w796:bool, "ImageParameter"=w792:T93)  [unwired: 6 in, 1 out]
            n1134 = case shown="False" w796 {
              tunnel: w794 -> [w798 w828]
              tunnel: w795 -> [w827 _]
              tunnel: [w801 w828] -> w793
              tunnel: w792 -> [w820 _]
              tunnel: w791 -> [w823 _]
              tunnel: w790 -> [w822 _]
              tunnel: w788 -> [w813 _]
              frame False {
                w805 = T1 1 items=["1"=1, "5"=5, "10"=10, "25"=25, "50"=50, "100"=100, "250"=250, "500"=500, "1000"=1000, "2500"=2500, "5000"=5000] ("Value (Signaling)")
                n1135 = control-ref of="SW_Average"() -> (w806:refnum<vi>)
                n1136 = property class="Ring (strict)"(reference=w806, error in=w798) -> (reference out=w807:refnum<vi>, error out=w804:errorcluster, "Value"=w797:T1)
                n1137 = local read "Velocity(Micos)"() -> (w803:dbl)
                n1138 = Unbundle By Name(w820) -> ("Start Position"=w818:dbl[], "StepWidth"=w817:dbl[], "Dimension"=w816:i32[], "ScanSpeed"=w819:dbl)
                n1139 = property class="Ring (strict)"(reference=w807, error in=w804, "Val(Sgnl)"=w805) -> (reference out=w800:refnum<vi>, error out=w799:errorcluster)
                n1140 = property on="Sample Rate" class="DigNum (strict)"() -> ("Value"=w811:dbl)  [unwired: 2 in, 2 out]
                n1141 = property on="Trigger Delay" class="DigNum (strict)"() -> ("Value"=w810:dbl)  [unwired: 2 in, 2 out]
                n1142 = property on="Depth" class="DigNum (strict)"() -> ("Value"=w812:dbl)  [unwired: 2 in, 2 out]
                n1143 = Subtract(x=w812, y=64.0) -> (x-y=w809:dbl)
                n1144 = property on="Cali." class="Arr (strict)"() -> ("Value"=w815:dbl[])  [unwired: 2 in, 2 out]
                n1145 = Bundle By Name(cluster=T79 {"File Header"={"Start Position"=[], "StepWidth"=[], "Dimension"=[], "SpecLength"=0}, "ScanSpeed"=0.0, "HighSpeed"=0.0, "SampleRate"=0.0, "Rep.Rate (Hz)"=0.0, "TrigDelay"=0.0, "mzCali"=[], "KeepStill(ms)"=0, "SaveRaw"=FALSE} ("BeamProfiling_Params"), "File Header.SpecLength"=w809, "SampleRate"=w811, "TrigDelay"=w810, "mzCali"=w815, "File Header.Start Position"=w818, "File Header.StepWidth"=w817, "File Header.Dimension"=w816, "ScanSpeed"=w819, "HighSpeed"=w803) -> (w814:T79)
                n1146 = Unbundle By Name(w823) -> ("Micos"=w824:refnum<queue>)
                n1147 = call "MeanderCtrl_Dynamic,StageRefs.vi"("QueuesRef"=w823, "MotionStageRefs"=w824, "AppsRef"=w822, "subprog_Ref"=w813, "Params."=w814, "Laser_Ctrl"=w827, "error in"=w799, "HighSpeed"=w803, "LowSpeed"=w819) -> ("error out"=w825:errorcluster)  [unwired: 5 in, 1 out]
                n1148 = property on="Record" class="Bool (strict)"(error in=w825, "Val(Sgnl)"=FALSE) -> (error out=w802:errorcluster)  [unwired: 1 in, 1 out]
                n1149 = property class="Ring (strict)"(reference=w800, error in=w802, "Val(Sgnl)"=w797) -> (error out=w801:errorcluster)  [unwired: 1 out]
              }
              frame True {
              }
            }
          }
          frame "DepthProfiling(3D)" {
            n1150 = global read "Position_Micos.vi" "Position(Micos)"() -> (w831:dbl[])
            n1151 = vi-ref "DepthProfiling_3D_Core.vi"() -> (w830:refnum<vi>)
            n1152 = call "CreateMeanderMask_3d.vi"("Rep. Rate (Hz)"=w829, "Start Position"=w831) -> ("Laser_Ctrl"=w837:bool, "start/end points"=w838:cluster{dbl, dbl, dbl}[][], "Canceled"=w839:bool, "ImageParameter"=w834:T93)  [unwired: 6 in]
            n1153 = case shown="False" w839 {
              tunnel: w838 -> [_ _]
              tunnel: w836 -> [w842 w871]
              tunnel: w837 -> [w870 _]
              tunnel: [w848 w871] -> w835
              tunnel: w834 -> [w863 _]
              tunnel: w833 -> [w866 _]
              tunnel: w832 -> [w865 _]
              tunnel: w830 -> [w855 _]
              frame False {
                w843 = T1 1 items=["1"=1, "5"=5, "10"=10, "25"=25, "50"=50, "100"=100, "250"=250, "500"=500, "1000"=1000, "2500"=2500, "5000"=5000] ("Value (Signaling)")
                n1154 = control-ref of="SW_Average"() -> (w845:refnum<vi>)
                n1155 = property class="Ring (strict)"(reference=w845, error in=w842) -> (reference out=w846:refnum<vi>, error out=w841:errorcluster, "Value"=w844:T1)
                n1156 = property class="Ring (strict)"(reference=w846, error in=w841, "Val(Sgnl)"=w843) -> (reference out=w847:refnum<vi>, error out=w840:errorcluster)
                n1157 = Unbundle By Name(w863) -> ("Start Position"=w861:dbl[], "StepWidth"=w860:dbl[], "Dimension"=w859:i32[], "ScanSpeed"=w862:dbl)
                n1158 = property on="Sample Rate" class="DigNum (strict)"() -> ("Value"=w853:dbl)  [unwired: 2 in, 2 out]
                n1159 = property on="Trigger Delay" class="DigNum (strict)"() -> ("Value"=w852:dbl)  [unwired: 2 in, 2 out]
                n1160 = property on="Depth" class="DigNum (strict)"() -> ("Value"=w854:dbl)  [unwired: 2 in, 2 out]
                n1161 = local read "Velocity(Micos)"() -> (w856:dbl)
                n1162 = Subtract(x=w854, y=64.0) -> (x-y=w851:dbl)
                n1163 = property on="Cali." class="Arr (strict)"() -> ("Value"=w858:dbl[])  [unwired: 2 in, 2 out]
                n1164 = Bundle By Name(cluster=T79 {"File Header"={"Start Position"=[], "StepWidth"=[], "Dimension"=[], "SpecLength"=0}, "ScanSpeed"=0.0, "HighSpeed"=0.0, "SampleRate"=0.0, "Rep.Rate (Hz)"=0.0, "TrigDelay"=0.0, "mzCali"=[], "KeepStill(ms)"=0, "SaveRaw"=FALSE} ("BeamProfiling_Params"), "File Header.SpecLength"=w851, "SampleRate"=w853, "TrigDelay"=w852, "mzCali"=w858, "File Header.Start Position"=w861, "File Header.StepWidth"=w860, "File Header.Dimension"=w859, "ScanSpeed"=w862, "HighSpeed"=w856) -> (w857:T79)
                n1165 = Unbundle By Name(w866) -> ("Micos"=w867:refnum<queue>)
                n1166 = call "MeanderCtrl_Dynamic,StageRefs.vi"("QueuesRef"=w866, "MotionStageRefs"=w867, "AppsRef"=w865, "subprog_Ref"=w855, "Params."=w857, "Laser_Ctrl"=w870, "error in"=w840, "HighSpeed"=w856, "LowSpeed"=w862) -> ("error out"=w868:errorcluster)  [unwired: 5 in, 1 out]
                n1167 = property on="Record" class="Bool (strict)"(error in=w868, "Val(Sgnl)"=FALSE) -> (error out=w849:errorcluster)  [unwired: 1 in, 1 out]
                n1168 = property class="Ring (strict)"(reference=w847, error in=w849, "Val(Sgnl)"=w844) -> (error out=w848:errorcluster)  [unwired: 1 out]
              }
              frame True {
              }
            }
          }
          frame "DepthProfile_RT" {
            n1169 = global read "Position_Micos.vi" "Position(Micos)"() -> (w875:dbl[])
            n1170 = vi-ref "DepthProfiling_Proc.vi"() -> (w878:refnum<vi>)
            n1171 = call "DepthProfile_Setup.vi"("RepRate (Hz)"=w872, "Start Position"=w875) -> ("Depth Profile Params."=w874:T95, "Canceled"=w876:bool, "Meander_Params."=w877:T77, "SaveRaw"=w873:bool)  [unwired: 6 in]
            n1172 = case shown="False" w876 {
              tunnel: w882 -> [w888 w922]
              tunnel: [w906 w922] -> w881
              tunnel: w877 -> [w889 _]
              tunnel: w880 -> [w890 _]
              tunnel: w879 -> [w903 _]
              tunnel: w878 -> [w896 _]
              tunnel: w874 -> [w895 _]
              tunnel: w873 -> [w886 _]
              frame False {
                n1173 = case "Save Raw File for offline processing" shown="True" w886 {
                  tunnel: w890 -> [_ w913]
                  tunnel: w889 -> [_ w912]
                  tunnel: w888 -> [w908 w911]
                  tunnel: [w908 w910] -> w887
                  frame False {
                  }
                  frame True {
                    n1174 = Unbundle By Name(w912) -> ("Start Position"=w917:dbl[], "StepWidth"=w916:dbl[], "Dimension"=w915:i32[])
                    n1175 = Unbundle By Name(w913) -> ("WriterCtrl"=w914:refnum<queue>)
                    n1176 = property on="Depth" class="DigNum (strict)"() -> ("Value"=w909:dbl)  [unwired: 2 in, 2 out]
                    n1177 = Bundle By Name(cluster=T77 {"Start Position"=[], "StepWidth"=[], "Dimension"=[], "SpecLength"=0} ("File Header"), "Start Position"=w917, "StepWidth"=w916, "Dimension"=w915, "SpecLength"=w909) -> (w918:T77)
                    n1178 = Bundle By Name(cluster=T68 {"State"=enum."SetHeader", "Params"=variant} ("element"), "Params"=w918) -> (w920:T68)
                    n1179 = Enqueue Element(queue=w914, element=w920, error in (no error)=w911) -> (error out=w910:errorcluster)  [unwired: 1 in, 2 out]
                  }
                }
                n1180 = property on="Depth" class="DigNum (strict)"() -> ("Value"=w884:dbl)  [unwired: 2 in, 2 out]
                n1181 = property on="Sample Rate" class="DigNum (strict)"() -> ("Value"=w885:dbl)  [unwired: 2 in, 2 out]
                n1182 = property on="Trigger Delay" class="DigNum (strict)"() -> ("Value"=w883:dbl)  [unwired: 2 in, 2 out]
                n1183 = Unbundle By Name(w895) -> ("HighSpeed"=w891:dbl, "RepRate (Hz)"=w892:dbl, "z-depth (ms)"=w893:u32)  [unwired: 1 out]
                n1184 = Unbundle By Name(w889) -> ("Start Position"=w901:dbl[], "StepWidth"=w900:dbl[], "Dimension"=w899:i32[])
                n1185 = property on="Cali." class="Arr (strict)"() -> ("Value"=w898:dbl[])  [unwired: 2 in, 2 out]
                n1186 = Bundle By Name(cluster=T79 {"File Header"={"Start Position"=[], "StepWidth"=[], "Dimension"=[], "SpecLength"=0}, "ScanSpeed"=0.0, "HighSpeed"=0.0, "SampleRate"=0.0, "Rep.Rate (Hz)"=0.0, "TrigDelay"=0.0, "mzCali"=[], "KeepStill(ms)"=0, "SaveRaw"=FALSE} ("BeamProfiling_Params"), "File Header.SpecLength"=w884, "SampleRate"=w885, "TrigDelay"=w883, "mzCali"=w898, "SaveRaw"=w886, "File Header.Start Position"=w901, "File Header.StepWidth"=w900, "File Header.Dimension"=w899, "ScanSpeed"=w891, "HighSpeed"=w891, "Rep.Rate (Hz)"=w892, "KeepStill(ms)"=w893) -> (w897:T79)
                n1187 = Unbundle By Name(w890) -> ("Micos"=w904:refnum<queue>)
                n1188 = call "MeanderCtrl_Dynamic,StageRefs.vi"("QueuesRef"=w890, "MotionStageRefs"=w904, "AppsRef"=w903, "subprog_Ref"=w896, "Params."=w897, "Laser_Ctrl"=TRUE, "error in"=w887, "HighSpeed"=w891, "LowSpeed"=w891) -> ("error out"=w905:errorcluster)  [unwired: 5 in, 1 out]
                n1189 = property on="Record" class="Bool (strict)"(error in=w905, "Val(Sgnl)"=FALSE) -> (error out=w906:errorcluster)  [unwired: 1 in, 1 out]
              }
              frame True {
              }
            }
          }
          frame "DepthProfiling" {
            n1190 = global read "Position_Micos.vi" "Position(Micos)"() -> (w925:dbl[])
            n1191 = call "DepthProfile_Setup.vi"("RepRate (Hz)"=w923, "Start Position"=w925) -> ("Depth Profile Params."=w924:T95, "Canceled"=w931:bool, "Meander_Params."=w928:T77)  [unwired: 6 in, 1 out]
            n1192 = case shown="False" w931 {
              tunnel: w930 -> [w942 w955]
              tunnel: [w945 w955] -> w929
              tunnel: w928 -> [w949 _]
              tunnel: w927 -> [w939 _]
              tunnel: w926 -> [w938 _]
              tunnel: w924 -> [w936 _]
              frame False {
                n1193 = Unbundle By Name(w949) -> ("Start Position"=w948:dbl[], "StepWidth"=w947:dbl[], "Dimension"=w946:i32[])
                n1194 = property on="Depth" class="DigNum (strict)"() -> ("Value"=w932:dbl)  [unwired: 2 in, 2 out]
                n1195 = Unbundle By Name(w939) -> ("WriterCtrl"=w940:refnum<queue>)
                n1196 = Bundle By Name(cluster=T77 {"Start Position"=[], "StepWidth"=[], "Dimension"=[], "SpecLength"=0} ("File Header"), "Start Position"=w948, "StepWidth"=w947, "Dimension"=w946, "SpecLength"=w932) -> (w950:T77)
                n1197 = Unbundle By Name(w936) -> ("SamplingPos."=w934:cluster{"x":dbl, "y":dbl, "z":dbl}[][], "HighSpeed"=w935:dbl, "z-depth (ms)"=w933:u32)  [unwired: 1 out]
                n1198 = Bundle By Name(cluster=T68 {"State"=enum."SetHeader", "Params"=variant} ("element"), "Params"=w950) -> (w952:T68)
                n1199 = Enqueue Element(queue=w940, element=w952, error in (no error)=w942) -> (error out=w943:errorcluster)  [unwired: 1 in, 2 out]
                n1200 = Unbundle By Name(w939) -> ("Micos"=w941:refnum<queue>)
                n1201 = call "MeanderCtrl_3d_StageRefs.vi"("QueuesRef"=w939, "MotionStageRefs"=w941, "AppsRef"=w938, "start/end points"=w934, "Laser_Ctrl"=TRUE, "error in"=w943, "HighSpeed"=w935, "ScanSpeed"=w935, "KeepStill"=w933) -> ("error out"=w944:errorcluster)  [unwired: 4 in, 2 out]
                n1202 = property on="Record" class="Bool (strict)"(error in=w944, "Val(Sgnl)"=FALSE) -> (error out=w945:errorcluster)  [unwired: 1 in, 1 out]
              }
              frame True {
              }
            }
          }
          frame "Set_2PulseDelay" {
            n1203 = Unbundle By Name(w974) -> ("ESP300"=w972:refnum<queue>)
            n1204 = Bundle By Name(cluster=T80 {"MotionStageRefs"=refnum, "Axis#"=0, "Delay(ps)"=0.0, "ZeroDelay_Offset"=0.0} ("Params."), "MotionStageRefs"=w972, "Delay(ps)"="DP_Delay (ps)", "ZeroDelay_Offset"="ZeroDelayPos") -> (w971:T80)
            n1205 = control-ref of="Destination(ESP)"() -> (w965:refnum<vi>)
            n1206 = property class="Arr (strict)"(reference=w965) -> (reference out=w964:refnum<vi>, error out=w957:errorcluster, "Value"=w960:dbl[])  [unwired: 1 in]
            n1207 = call "Set_DoublePulse_Delay.vi"("error in"=w969, "WaitForReady"=TRUE, "InputParams."=w971) -> ("error out"=w966:errorcluster, "DP_StagePos."=w961:variant)  [unwired: 7 in]
            n1208 = Variant To Data(error in=w957, type=w960, Variant=w961) -> (data=w959:dbl[], error out=w958:errorcluster)
            n1209 = Replace Array Subset(array=w960, new element=w959, index=0) -> (w963:dbl[])
            n1210 = property class="Arr (strict)"(reference=w964, error in=w958, "Value"=w963) -> (error out=w956:errorcluster)  [unwired: 1 out]
            n1211 = call <vilib>:"Clear Errors.vi"("error in (no error)"=w956) -> ()  [unwired: 6 in, 1 out]
          }
          frame "DelayScan" {
            n1212 = local read "ZeroDelayPos"() -> (w976:dbl)
            n1213 = global read "Position_Micos.vi" "Position(Micos)"() -> (w980:dbl[])
            n1214 = Unbundle By Name(w979) -> ("ESP300"=w978:refnum<queue>)
            n1215 = call "DoublePulse_Delay_Scan_Setup.vi"("Rep. Rate (Hz)"=w975, "ZeroDelayPos"=w976, "Start Position"=w980, "ESP300"=w978) -> ("Laser_Ctrl"=w985:bool, "start/end points"=w986:cluster{dbl, dbl, dbl}[][], "Canceled"=w987:bool, "SecondaryParams"=w977:variant[], "ImageParameter"=w982:T93)  [unwired: 3 in]
            n1216 = case shown="False" w987 {
              tunnel: w986 -> [w1011 _]
              tunnel: w984 -> [w998 w1012]
              tunnel: w985 -> [w1010 _]
              tunnel: [w1001 w1012] -> w983
              tunnel: w982 -> [w994 _]
              tunnel: w979 -> [w992 _]
              tunnel: w981 -> [w996 _]
              tunnel: w977 -> [w989 _]
              frame False {
                n1217 = Unbundle By Name(w994) -> ("ScanSpeed"=w993:dbl)
                n1218 = local read "Velocity(Micos)"() -> (w995:dbl)
                n1219 = Unbundle By Name(w994) -> ("Start Position"=w1004:dbl[], "StepWidth"=w1003:dbl[], "Dimension"=w1002:i32[])
                n1220 = property on="Depth" class="DigNum (strict)"() -> ("Value"=w988:dbl)  [unwired: 2 in, 2 out]
                n1221 = Unbundle By Name(w992) -> ("WriterCtrl"=w997:refnum<queue>)
                n1222 = Bundle By Name(cluster=T77 {"Start Position"=[], "StepWidth"=[], "Dimension"=[], "SpecLength"=0} ("File Header"), "Start Position"=w1004, "StepWidth"=w1003, "Dimension"=w1002, "SpecLength"=w988) -> (w1005:T77)
                n1223 = Bundle By Name(cluster=T68 {"State"=enum."SetHeader", "Params"=variant} ("element"), "Params"=w1005) -> (w1007:T68)
                n1224 = Enqueue Element(queue=w997, element=w1007, error in (no error)=w998) -> (error out=w999:errorcluster)  [unwired: 1 in, 2 out]
                n1225 = Unbundle By Name(w992) -> ("Micos"=w991:refnum<queue>)
                n1226 = vi-ref "Set_DoublePulse_Delay.vi"() -> (w990:refnum<vi>)
                n1227 = call "MeanderCtrl_3d_StageRefs.vi"("QueuesRef"=w992, "MotionStageRefs"=w991, "AppsRef"=w996, "SecondaryVI_Ref"=w990, "SecondaryParams"=w989, "start/end points"=w1011, "Laser_Ctrl"=w1010, "error in"=w999, "HighSpeed"=w995, "ScanSpeed"=w993) -> ("error out"=w1000:errorcluster)  [unwired: 3 in, 2 out]
                n1228 = property on="Record" class="Bool (strict)"(error in=w1000, "Val(Sgnl)"=FALSE) -> (error out=w1001:errorcluster)  [unwired: 1 in, 1 out]
              }
              frame True {
              }
            }
          }
          frame "Save Settings" {
            n1229 = feedback #9(path "" ("selected path")) -> (w1016:path)
            n1230 = Strip Path(path=w1016) -> (stripped path=w1018:path, name=w1017:string)
            n1231 = call "File Dialog4"("start path"=w1018, "default name"=w1017, "pattern (all files)"="*.conf.json", "pattern label"="Json Configuration Files") -> ("selected path"=w1020:path, "cancelled"=w1021:bool)  [unwired: 8 in, 2 out]
            n1232 = feedback-in #9(w1020) -> ()
            n1233 = case shown="False" w1021 {
              tunnel: w1013 -> [w1022 _]
              frame False {
                n1234 = call "SaveConfigs_toFile.vi"("Configuration"=w1022) -> ()  [unwired: 11 in]
              }
              frame True {
              }
            }
          }
          frame "EnergyCalibration" {
            n1235 = Unbundle By Name(w1024) -> ("ESP300"=w1023:refnum<queue>)
            n1236 = call "Acquire_EnergyCalibrationCurve.vi"("Queue in"=w1023) -> ()  [unwired: 10 in, 1 out]
          }
          frame "Quit" {
            n1237 = Unbundle By Name(w1058) -> ("SRS DG535"=w1045:refnum<queue>, "BNC"=w1057:refnum<queue>, "Feedback"=w1056:refnum<queue>, "ESP300"=w1055:refnum<queue>, "Micos"=w1054:refnum<queue>, "SDG_ii"=w1053:refnum<queue>, "EPM2000"=w1035:refnum<queue>, "NI-USB_DAQmx"=w1052:refnum<queue>, "MainDAQCoreQueue"=w1051:refnum<queue>, "WriterCtrl"=w1050:refnum<queue>)  [unwired: 1 out]
            n1238 = Release Queue(queue=w1068, error in (no error)=w1069) -> ()  [unwired: 1 in, 3 out]
            n1239 = Enqueue Element(queue=w1050, element=T68 {"State"=enum."QuitProg.", "Params"=variant}) -> ()  [unwired: 2 in, 3 out]
            n1240 = Enqueue Element(queue=w1051, element=T60 {"DWF States"=enum."Quit", "Variant"=variant}) -> ()  [unwired: 2 in, 3 out]
            n1241 = global write "QuitProg.vi" "QuitProg."(TRUE ("QuitProg.")) -> ()
            n1242 = Enqueue Element(queue=w1052, element=T84 {"State"=enum."Quit", "Para."=variant}) -> ()  [unwired: 2 in, 3 out]
            n1243 = Enqueue Element(queue=w1035, element=T82 {"State"=enum."Close", "Parameter"=0.0}) -> (queue out=w1046:refnum<queue>)  [unwired: 2 in, 2 out]
            n1244 = Enqueue Element(queue=w1046, element=T82 {"State"=enum."Quit", "Parameter"=0.0}) -> ()  [unwired: 2 in, 3 out]
            n1245 = Enqueue Element(queue=w1053, element=T70 {"State"=enum."Tun OFF", "Parameter"=0.0}) -> (queue out=w1060:refnum<queue>)  [unwired: 2 in, 2 out]
            n1246 = Enqueue Element(queue=w1060, element=T70 {"State"=enum."Close", "Parameter"=0.0}) -> (queue out=w1048:refnum<queue>)  [unwired: 2 in, 2 out]
            n1247 = Enqueue Element(queue=w1054, element=T74 {"State"=enum."STOP", "Params."=variant}) -> (queue out=w1029:refnum<queue>)  [unwired: 2 in, 2 out]
            n1248 = Enqueue Element(queue=w1045, element=T81 {"State"=enum."Stop", "Para."=variant}) -> (queue out=w1041:refnum<queue>, error out=w1034:errorcluster)  [unwired: 2 in, 1 out]
            n1249 = Enqueue Element(queue=w1048, element=T70 {"State"=enum."Quit", "Parameter"=0.0}) -> ()  [unwired: 2 in, 3 out]
            n1250 = Enqueue Element(queue=w1057, element=T83 {"State"=enum."Close", "Para."=variant}) -> (queue out=w1063:refnum<queue>)  [unwired: 2 in, 2 out]
            n1251 = Enqueue Element(queue=w1063, element=T83 {"State"=enum."Quit", "Para."=variant}) -> ()  [unwired: 2 in, 3 out]
            n1252 = Bundle By Name(cluster=T74 {"State"=enum."MotorEnable(1)", "Params."=variant} ("element"), "Params."=FALSE) -> (w1027:T74)
            n1253 = Enqueue Element(queue=w1041, element=T81 {"State"=enum."Close", "Para."=variant}, error in (no error)=w1034) -> (queue out=w1040:refnum<queue>, error out=w1033:errorcluster)  [unwired: 1 in, 1 out]
            n1254 = Enqueue Element(queue=w1029, element=w1027) -> (queue out=w1028:refnum<queue>)  [unwired: 2 in, 2 out]
            n1255 = Enqueue Element(queue=w1028, element=T74 {"State"=enum."Close", "Params."=variant}) -> (queue out=w1036:refnum<queue>)  [unwired: 2 in, 2 out]
            n1256 = Enqueue Element(queue=w1040, element=T81 {"State"=enum."Quit", "Para."=variant}, error in (no error)=w1033) -> (error out=w1032:errorcluster)  [unwired: 1 in, 2 out]
            n1257 = Enqueue Element(queue=w1036, element=T74 {"State"=enum."Quit", "Params."=variant}) -> ()  [unwired: 2 in, 3 out]
            n1258 = call <vilib>:"Clear Errors.vi"("error in (no error)"=w1032) -> ()  [unwired: 6 in, 1 out]
            n1259 = Enqueue Element(queue=w1055, element=T74 {"State"=enum."Quit", "Params."=variant}) -> ()  [unwired: 2 in, 3 out]
            n1260 = Release Queue(queue=w1056) -> ()  [unwired: 2 in, 3 out]
          }
          frame "Check_AppsLock" {
            # "No need"
          }
          frame Default {
            n1261 = property on="Property Node" class="Str"(reference=w1072) -> (reference out=w1075:refnum<vi>, "Value"=w1076:string)  [unwired: 1 in, 1 out]
            n1262 = Format Into String(format string="%s", initial string="\nUnsupported function:", w1079) -> (resulting string=w1074:string)  [unwired: 1 in, 1 out]
            n1263 = Concatenate Strings(w1076, w1074) -> (w1073:string)
            n1264 = property on="Property Node" class="Str"(reference=w1075, "Value"=w1073) -> ()  [unwired: 1 in, 2 out]
          }
        }
        n1265 = call <userlib>:"ErrorLog.vi"("error in (no error)"=w531) -> ("error out"=w523:errorcluster)  [unwired: 10 in]
        n1266 = call <vilib>:"Release Semaphore.vi"("error in (no error)"=w523, "semaphore"=w524) -> ("error out"=w522:errorcluster)  [unwired: 4 in, 1 out]
      }
      n1267 = Merge Errors(w223, w224, w225, w226, w227, w228, w229) -> (w222:errorcluster)
      n1268 = Merge Errors(w165, w169, w168) -> (w164:errorcluster)
      n1269 = Release Queue(queue=w171, error in (no error)=w164) -> (error out=w172:errorcluster)  [unwired: 1 in, 2 out]
      n1270 = Release Queue(queue=w173, error in (no error)=w172) -> (error out=w166:errorcluster)  [unwired: 1 in, 2 out]
      n1271 = Release Queue(queue=w162, error in (no error)=w166) -> (error out=w167:errorcluster)  [unwired: 1 in, 2 out]
      n1272 = Release Queue(queue=w163, error in (no error)=w167) -> (error out=w170:errorcluster)  [unwired: 1 in, 2 out]
      n1273 = Merge Errors(w222, w230, w170) -> (w221:errorcluster)
    }
  }
  n1274 = Release Queue(queue=w71, error in (no error)=w70) -> (error out=w54:errorcluster)  [unwired: 1 in, 2 out]
  n1275 = Release Queue(queue=w68, error in (no error)=w54) -> (error out=w69:errorcluster)  [unwired: 1 in, 2 out]
  n1276 = Release Queue(queue=w67, error in (no error)=w69) -> (error out=w65:errorcluster)  [unwired: 1 in, 2 out]
  n1277 = Release Queue(queue=w66, error in (no error)=w65) -> (error out=w63:errorcluster)  [unwired: 1 in, 2 out]
  n1278 = Release Queue(queue=w64, error in (no error)=w63) -> (error out=w60:errorcluster)  [unwired: 1 in, 2 out]
  n1279 = Release Queue(queue=w61, error in (no error)=w60) -> (error out=w59:errorcluster)  [unwired: 1 in, 2 out]
  n1280 = Release Queue(queue=w62, error in (no error)=w59) -> (error out=w58:errorcluster)  [unwired: 1 in, 2 out]
  n1281 = call <vilib>:"General Error Handler.vi"("type of dialog (OK msg:1)"=w57, "error in (no error)"=w58, "[exception action] (none:0)"=w56, "[exception code]"=1) -> ()  [unwired: 7 in, 5 out]
